vi "BeamPointing General v08.vi"() -> ()   [LabVIEW 2013]
doc: "This example illustrates how to perform a continuous acquisition with a USB camera."
uses:
  <vilib>/vision/Image Controls.llb/IMAQ Image.ctl
  <vilib>/userdefined/High Color/IMAQdx.ctl
  shared programs/GUI_Template/GUI_master/tcp_new_data_event.ctl
  shared programs/GUI_Template/GUI_master/tcp new data cluster.ctl
  Add ROI Offset ImgData.vi
  Add Or Replace Coord Array.vi
  Add Or Replace Img Array.vi
  Add ROI Offset RectFilter.vi
  Add Or Replace String Array.vi
  <vilib>/regexp/Match Regular Expression.xnode
  <vilib>/vision/NI_Vision_Development_Module.lvlib
  <resource>/objmgr/IMAQImage.rc
  <vilib>/Analysis/NI_AALBase.lvlib
  <vilib>/Analysis/NI_AALPro.lvlib
panel:
  out "image::1":T1(plugin-control) caption="Mode1"
  out "image::4":T1(plugin-control) caption="Mode1"
  out "image::5":T1(plugin-control) caption="Mode1"
  out "image::6":T1(plugin-control) caption="Mode1"
  out "image::7":T1(plugin-control) caption="Mode1"
  out "image::8":T1(plugin-control) caption="Mode1"
  out "GUIdevice 5":string="M1Cam"
  out "GUIdevice 4":string="M1Cam"
  out "GUIdevice 7":string="M1Cam"
  out "GUIdevice 6":string="M1Cam"
  out "GUIdevice 8":string="M1Cam"
  out "GUIdevice 9":string="M1Cam"
  out "image::9":T1(plugin-control) caption="Mode1"
  out "GUIdevice 3":string="M1Cam"
  out "GUIdevice 1":string="M1Cam"
  out "GUIdevice 2":string="M1Cam"
  out "image::2":T1(plugin-control) caption="Mode1"
  out "image::3":T1(plugin-control) caption="Mode1"
  out "error IO 2":errorcluster
  in  "insert tag":bool=TRUE
  out "tcp data event":T2
  in  "image prefix 2":string="gbpimage"
  in  "newMC":bool=TRUE
  out "configarraychanged":bool
  in  "Stop 2":bool
  out "image names":string[](array[string])
  out "TCP IDs":refnum<k5>[](array[refnum])
  out "Image Dst Out":T1
  in  "recenter":bool
  out "Beam Detected":bool
  out "Move Y":bool
  out "Move X":bool
  in  "LoopMode":bool caption="Mode"
  in  "rescale":bool=TRUE
  in  "Step Size":u16=5
  in  "Feedback":bool
  out "MoveInProgress":bool caption="Move In Progress"
  in  "USB cameras":i32(listbox)=1 caption="Select Camera"
  in  "Manual Move":T3={"Down"=FALSE, "Up"=FALSE, "Right"=FALSE, "Left"=FALSE, "APulses X"=200, "APulses Y"=200, "StopButton"=FALSE}
  out "Status":string
  in  "Internal controls and indicators":T4(tab)
  out "grab loop i":i32=4
  out "Image client connect errors":errorcluster[](array[cluster])
  out "Image client grab errors":errorcluster[](array[cluster])=[{"status"=TRUE, "code"=56, "source"="UDP Read in GrabImageUDP.vi->BeamPointing General v03.vi"}, {"status"=TRUE, "code"=56, "source"="UDP Read in GrabImageUDP.vi->BeamPointing General v03.vi"}, {"status"=TRUE, "code"=56, "source"="UDP Read in GrabImageUDP.vi->BeamPointing General v03.vi"}, {"status"=TRUE, "code"=56, "source"="UDP Read in GrabImageUDP.vi->BeamPointing General v03.vi"}, {"status"=TRUE, "code"=56, "source"="UDP Read in GrabImageUDP.vi->BeamPointing General v03.vi"}, {"status"=TRUE, "code"=56, "source"="UDP Read in GrabImageUDP.vi->BeamPointing General v03.vi"}]
  out "Current ImageServer":cluster{"IPAddress":string, "Port":i32}={"IPAddress"="234.5.6.8", "Port"=58445}
  out "Ann. Images":T1[](array[typedef])=["imageserver0", "imageserver1", "imageserver2", "imageserver3", "imageserver4", "imageserver5"]
  in  "Tab Control 2":enum32{"Image saving", "stats", "TCP", "cams"}(tab)=enum."cams"
  in  "Boolean":bool
  in  "Base Directory":path
  out "SaveImgError":errorcluster
  in  "SavePict":bool
  out "error CamS":errorcluster
  out "Switch Time":u32=200
  out "one loop":u32=130
  out "# imgs in buffer":i32=5
  out "ImgBufferSize":i32=5
  out "AcqTime":u32=610845
  out "State":i32=12
  out "Main processing loop i":i32=3683
  out "TCPconnecAnswer":bool=TRUE
  out "TCPconnecCmd":bool=TRUE
  out "error close connect":errorcluster
  in  "Remove Camera":bool
  in  "Mirror List Path":path=path "Z:/Software/control-common/Configuration files/DeviceList100TW.xml"
  out "XML Config File Path":path=path "Z:/Software/control-common/Configuration files/ConfigFile_192_168_10_184.xml"
  in  "USB/RS170 cams":bool=TRUE
  in  "Add Camera":bool
  out "# of cams":i32=6
  in  "# Channels on Ontrak":i32
  in  "Corr":bool[](array[boolean])=[FALSE, FALSE, FALSE, FALSE, FALSE, FALSE]
  out "Det":bool[](array[boolean])
  out "error out":errorcluster
  out "IMAQ status":bool
  out "Avg Img Buffer":u8[][][](array[numeric])
  out "Switch in":u32=299180745
  out "MirrorList":string[][](array[string])
  out "Corrective Move XY":T5(array[cluster])
  out "Cameras Names":string[](array[string])=["Null", "Null", "Null", "Null", "Null", "Null"]
  out "Deviation":cluster{"Dev. X":sgl, "Dev. Y":sgl}={"Dev. X"=0.0, "Dev. Y"=-5.0} {"Dev. X" format="%.1f"; "Dev. Y" format="%.1f"}
  out "Buffer2":T1
  out "DownloadedImg":T1
  out "CurrentName":string="*100TW M10"
  out "XML errors":bool
  out "Image Odd Out":T1
  out "DeviceNames":string[](array[string])=["no-device", "GasJet", "Godzilla_M1", "Godzilla_M2", "Godzilla_M3", "Godzilla_M4", "Godzilla_M6", "Godzilla_M8_Steer", "Chihuahua_M1", "Chihuahua_M2", "Collider_M4", "Collider_M5", "Collider_M8 Translation s3c4", "HeaterBlue-M1", "HeaterBlue-M2", "HeaterBlue-M3", "THz OAP Down", "G Spot Camera", "G Spot Monitor", "C Spot Monitor", "p15c4-Free", "THz_M5", "THz_M7A & Xtal", "THz_M7B", "THz MIrror Top", "THz OAP Top", "p2s2c2-Free", "p2s2c3-Free", "p2s2c4-Free", "Heater_M0", "Heater_M4", "Heater_M5", "Ignitor Iris", "Ignitor_M4", "Collider_M6", "Collder_M7", "C Spot Camera", "p2s5c1-FREE", "p2s5c2-FREE", "p2s5c3-FREE", "p2c5c4-FREE", "*100TW M9", "*100TW M10", "*100TW Preamp Up", "*100TW Input Preamp2", "*100TW Output Preamp2", "*100TW M0", "*100TW M2", "*100TW M4", "*100TW M6", "*100TW M8", "*100TW M13", "*100TW M20", "*100TW M22", "*100TW M23", "no pico", "no pico", "no pico", "mobile no ir", "regen out-salad#1", "preamp in-salad#2", "XPW 1", "blue periscope regen", "godzilla 1st", "godzilla IN", "Chihuahua IN", "Chihuahua 1st", "??XPW pico2", "Preamp 3rd pass", "Blue regen out"]
  out "size(s)":i32[](array[numeric])=[964, 1288]
  out "Iteration":u32
  in  "Onward":bool=TRUE
  out "Ellipse edges":cluster{"X":sgl, "Y":sgl}[](array[cluster])
  out "Buffer":T1
  out "Output Img":T1
  out "Reference Img":T1
  out "Background Img":T1
  out "counter":i32
  out "First step":bool
  out "IMAQ Session":refnum<k11>
  out "IMAQ Session Array":refnum<k11>[](array[refnum])
  out "Display Current":bool=TRUE
  out "Region of Interest":i32[](array[numeric])
  out "Acq Img":T1
  out "MoveInProgressTimeIN":u32=296721656
  out "IMAQdx Session":T6="cam2"
  out "start":u32=299180614
  out "Avg Deviation":cluster{sgl, sgl}={0.0, -5.0}
  out "InProgress":string[](array[string])
  out "Centroid Avg Buffer":cluster{"X Centroid":sgl, "Y Centroid":sgl}[](array[cluster])=[{"X Centroid"=343.0, "Y Centroid"=203.0}, {"X Centroid"=301.0, "Y Centroid"=181.0}, {"X Centroid"=334.0, "Y Centroid"=201.0}, {"X Centroid"=289.0, "Y Centroid"=154.0}, {"X Centroid"=319.0, "Y Centroid"=232.0}]
  out "Img Buffer":T1[](array[typedef])=["Buffer0", "Buffer1", "Buffer2", "Buffer3", "Buffer4"]
  out "OpenTime":u32=298569900
  out "CloseCam":bool=TRUE
  out "RunON/OFF":bool
  out "last move time":u32=281970384
  out "DeviationArray":cluster{"X Centroid":sgl, "Y Centroid":sgl}[](array[cluster])
  out "ConnectArray":T7(array[cluster])=[{"IPaddress"="192.168.10.34", "Port"=63420, "connection ID"=refnum, "TCP error"={"status"=FALSE, "code"=0, "source"=""}}, {"IPaddress"="192.168.10.184", "Port"=63430, "connection ID"=refnum, "TCP error"={"status"=FALSE, "code"=0, "source"=""}}]
  out "Raw images":T1[](array[typedef])=["imageserver0", "imageserver1", "imageserver2", "imageserver3", "imageserver4", "imageserver5"]
  in  "XML Config File Path 2":path=path "H:/Software/control-common/Configuration files/ConfigFile_192_168_10_184.xml"
  out "AddCameraCluster":T8={"Add?"=FALSE, "Channel"=6, "Device Name"="no-device"}
  out "RemoveCameraCluster":cluster{"Remove?":bool, "number":i32}={"Remove?"=FALSE, "number"=-1}
  out "NewAvg":bool
  out "Thresh Img":T1
  out "Avg Img":T1
  out "UDP connect array":refnum<k16>[](array[refnum])
  out "really save cfg?":bool
  out "Buffer3":T1
  out "CamConfigArray":T9(array[cluster])=[{"ID"=64.0, "Name"="*100TW M8", "DeviceID"={"Slot Connector"=24, "IP Adress"="192.168.10.34", "Port"=63420, "Type"="picodriver"}, "CorrectConfig Cluster"={"Detection Parameters"={"Contrast"=0, "Treshold"=0, "Max Intensity"=0, "Max Intensity%"=0, "Rx"=0, "Ry"=0, "R%"=0.0}, "Reverse"={"Reverse X"=FALSE, "Reverse Y"=FALSE}, "Target"={"X Target"=0.0, "Y Target"=0.0}, "Region of Interest"=[0, 0, 0, 0], "Correction Parameters"={"X"=0.0, "Y"=0.0, "Movement Type"=0}, "Acquisition Parameters"={"Brightness"=0.0, "Contrast"=0.0, "Saturation"=0.0, "White level"=0.0}, "Background Path"=path "", "Reference Path"=path "", "XCalibration"=[], "YCalibration"=[]}, "Ontrak Channel"=0, "IMAQdx Session 2"="cam2", "ImageServer"={"IPAddress"="234.5.6.8", "Port"=58450}}, {"ID"=55.0, "Name"="*100TW M9", "DeviceID"={"Slot Connector"=31, "IP Adress"="192.168.10.34", "Port"=63420, "Type"="picodriver"}, "CorrectConfig Cluster"={"Detection Parameters"={"Contrast"=0, "Treshold"=0, "Max Intensity"=0, "Max Intensity%"=0, "Rx"=0, "Ry"=0, "R%"=0.0}, "Reverse"={"Reverse X"=FALSE, "Reverse Y"=FALSE}, "Target"={"X Target"=631.0, "Y Target"=473.0}, "Region of Interest"=[0, 0, 0, 0], "Correction Parameters"={"X"=0.0, "Y"=0.0, "Movement Type"=0}, "Acquisition Parameters"={"Brightness"=0.0, "Contrast"=0.0, "Saturation"=0.0, "White level"=0.0}, "Background Path"=path "", "Reference Path"=path "", "XCalibration"=[], "YCalibration"=[]}, "Ontrak Channel"=0, "IMAQdx Session 2"="cam2", "ImageServer"={"IPAddress"="234.5.6.8", "Port"=58444}}, {"ID"=56.0, "Name"="*100TW M10", "DeviceID"={"Slot Connector"=32, "IP Adress"="192.168.10.34", "Port"=63420, "Type"="picodriver"}, "CorrectConfig Cluster"={"Detection Parameters"={"Contrast"=53, "Treshold"=53, "Max Intensity"=255, "Max Intensity%"=80, "Rx"=116, "Ry"=92, "R%"=50.0}, "Reverse"={"Reverse X"=FALSE, "Reverse Y"=TRUE}, "Target"={"X Target"=334.0, "Y Target"=206.0}, "Region of Interest"=[0, 0, 0, 0], "Correction Parameters"={"X"=100.0, "Y"=100.0, "Movement Type"=0}, "Acquisition Parameters"={"Brightness"=0.0, "Contrast"=0.0, "Saturation"=0.0, "White level"=0.0}, "Background Path"=path "", "Reference Path"=path "", "XCalibration"=[], "YCalibration"=[]}, "Ontrak Channel"=0, "IMAQdx Session 2"="cam2", "ImageServer"={"IPAddress"="234.5.6.8", "Port"=58445}}, {"ID"=0.0, "Name"="*100TW M20", "DeviceID"={"Slot Connector"=1, "IP Adress"="192.168.10.184", "Port"=63430, "Type"="picodriver"}, "CorrectConfig Cluster"={"Detection Parameters"={"Contrast"=66, "Treshold"=66, "Max Intensity"=255, "Max Intensity%"=80, "Rx"=30, "Ry"=30, "R%"=50.0}, "Reverse"={"Reverse X"=TRUE, "Reverse Y"=TRUE}, "Target"={"X Target"=284.6373, "Y Target"=160.1435}, "Region of Interest"=[0, 0, 0, 0], "Correction Parameters"={"X"=20.0, "Y"=20.0, "Movement Type"=0}, "Acquisition Parameters"={"Brightness"=0.0, "Contrast"=0.0, "Saturation"=0.0, "White level"=0.0}, "Background Path"=path "", "Reference Path"=path "", "XCalibration"=[{-23000.0, -242.0}, {-22000.0, -229.0}, {-21000.0, -215.0}, {-20000.0, -203.0}, {-19000.0, -192.0}, {-18000.0, -182.0}, {-17000.0, -172.0}, {-16000.0, -162.0}, {-15000.0, -153.0}, {-14000.0, -141.0}, {-13000.0, -126.0}, {-12000.0, -105.0}, {-11000.0, -77.0}, {-10000.0, -44.0}, {0.0, 4.0}, {11000.0, 98.0}, {12000.0, 109.0}, {13000.0, 119.0}, {14000.0, 130.0}, {15000.0, 140.0}, {16000.0, 151.0}, {17000.0, 161.0}, {18000.0, 171.0}, {19000.0, 182.0}, {20000.0, 193.0}, {21000.0, 205.0}, {22000.0, 217.0}, {23000.0, 229.0}], "YCalibration"=[{-23000.0, 196.0}, {-22000.0, 189.0}, {-21000.0, 182.0}, {-20000.0, 174.0}, {-19000.0, 164.0}, {-18000.0, 153.0}, {-17000.0, 141.0}, {-16000.0, 133.0}, {-15000.0, 126.0}, {-14000.0, 117.0}, {-13000.0, 105.0}, {-12000.0, 90.0}, {-11000.0, 69.0}, {-10000.0, 42.0}, {0.0, -4.0}, {11000.0, -96.0}, {12000.0, -99.0}, {13000.0, -101.0}, {14000.0, -103.0}, {15000.0, -109.0}, {16000.0, -118.0}, {17000.0, -129.0}, {18000.0, -143.0}, {19000.0, -155.0}, {20000.0, -166.0}, {21000.0, -174.0}, {22000.0, -181.0}, {23000.0, -187.0}]}, "Ontrak Channel"=0, "IMAQdx Session 2"="cam2", "ImageServer"={"IPAddress"="234.5.6.8", "Port"=58443}}, {"ID"=12.0, "Name"="*100TW M22", "DeviceID"={"Slot Connector"=3, "IP Adress"="192.168.10.184", "Port"=63430, "Type"="picodriver"}, "CorrectConfig Cluster"={"Detection Parameters"={"Contrast"=59, "Treshold"=59, "Max Intensity"=255, "Max Intensity%"=80, "Rx"=47, "Ry"=33, "R%"=50.0}, "Reverse"={"Reverse X"=FALSE, "Reverse Y"=TRUE}, "Target"={"X Target"=319.0, "Y Target"=219.0}, "Region of Interest"=[0, 0, 0, 0], "Correction Parameters"={"X"=10000.0, "Y"=10000.0, "Movement Type"=0}, "Acquisition Parameters"={"Brightness"=0.0, "Contrast"=0.0, "Saturation"=0.0, "White level"=0.0}, "Background Path"=path "", "Reference Path"=path "", "XCalibration"=[], "YCalibration"=[]}, "Ontrak Channel"=0, "IMAQdx Session 2"="cam2", "ImageServer"={"IPAddress"="234.5.6.8", "Port"=58446}}, {"ID"=12.0, "Name"="*100TW M23", "DeviceID"={"Slot Connector"=4, "IP Adress"="192.168.10.184", "Port"=63430, "Type"="picodriver"}, "CorrectConfig Cluster"={"Detection Parameters"={"Contrast"=11, "Treshold"=11, "Max Intensity"=255, "Max Intensity%"=90, "Rx"=180, "Ry"=110, "R%"=50.0}, "Reverse"={"Reverse X"=FALSE, "Reverse Y"=TRUE}, "Target"={"X Target"=303.0, "Y Target"=342.0}, "Region of Interest"=[0, 0, 0, 0], "Correction Parameters"={"X"=0.0, "Y"=0.0, "Movement Type"=0}, "Acquisition Parameters"={"Brightness"=0.0, "Contrast"=0.0, "Saturation"=0.0, "White level"=0.0}, "Background Path"=path "", "Reference Path"=path "", "XCalibration"=[], "YCalibration"=[]}, "Ontrak Channel"=0, "IMAQdx Session 2"="cam2", "ImageServer"={"IPAddress"="234.5.6.8", "Port"=58442}}] {"CorrectConfig Cluster"."Acquisition Parameters"."White level" scale=0.3..1.26 scale format="%#_2f"; "CorrectConfig Cluster"."Acquisition Parameters"."Saturation" scale=0.5..1.5 scale format="%#_3f"; "CorrectConfig Cluster"."Acquisition Parameters"."Contrast" scale=0.4..1.5 scale format="%#_3f"; "CorrectConfig Cluster"."Acquisition Parameters"."Brightness" scale=-50.0..50.0 scale format="%#_2f"; "CorrectConfig Cluster"."Correction Parameters"."Movement Type" items=["Step", "Proportionnal"]; "CorrectConfig Cluster"."Target"."X Target" format="%#_5g"; "CorrectConfig Cluster"."Target"."Y Target" format="%#_5g"; "CorrectConfig Cluster"."Detection Parameters"."Max Intensity%" max=100 step=1}
  out "Ellipse":T10 {"Minor Axis"."Point 2"."Y" format="%.2f"; "Minor Axis"."Point 2"."X" format="%.2f"; "Minor Axis"."Point 1"."Y" format="%.2f"; "Minor Axis"."Point 1"."X" format="%.2f"; "Major Axis"."Point 2"."Y" format="%.2f"; "Major Axis"."Point 2"."X" format="%.2f"; "Major Axis"."Point 1"."Y" format="%.2f"; "Major Axis"."Point 1"."X" format="%.2f"; "Center"."Y" format="%.2f"; "Center"."X" format="%.2f"}
  out "Avg Variation":cluster{"mean X":dbl, "mean Y":dbl}={"mean X"=nan, "mean Y"=nan} {"mean X" format="%#_4g"; "mean Y" format="%#_4g"}
  in  "Acquisition Parameters dx":T11 {"Parameter4" min=0.0 max=0.1 scale=0.0..0.1 scale format="%#_2f"; "Parameter3" min=0.0 max=3.0 scale=0.0..3.0 scale format="%#_3f"; "Parameter2" min=1.0 max=10.0 scale=1.0..10.0 scale format="%#_3f"; "Parameter1" min=1 max=1048576 step=1 scale=1.0..1048576.0}
  in  "set scales":bool
  out "Image Ports":i32[](array[numeric])
  out "Image IPs":string[](array[string])
  out "device associated":string
  in  "Background Path":path
  in  "Reference Path":path
  out "BestRects Cluster":T12={"PreviousCenter"={"X"=0.0, "Y"=0.0}, "CurrentCenter"={"X"=334.0, "Y"=201.0}}
  out "Default devices":string[](array[string])=["*100TW M8", "*100TW M9", "*100TW M10", "*100TW M20", "*100TW M22", "*100TW M23"]
  out "Img Size":i32[](array[numeric])=[0, 0, 1288, 964]
  out "RectFilter":T13={"Left"=257, "Top"=144, "Right"=399, "Bottom"=260, "Rotation"=10.484647750854492} {"Rotation" format="%.2f"; "Left" scale=0.0..1024.0; "Right" scale=0.0..1024.0}
  out "History XY Buffer":T14(array[cluster])
  out "ImgDataArray":T15(array[cluster])
  out "DeviceList":T16(array[cluster])=[{"ID"=0.0, "Name"="no-device", "DeviceID"={"Slot Connector"=0, "IP Adress"="Ipaddress", "Port"=0, "Type"="Type"}, "Detection Parameters"={"Contrast"=0, "Treshold"=0, "Max Intensity"=0, "Max Intensity%"=0, "Rx"=0, "Ry"=0, "R%"=0.0}, "Reverse"={"Reverse X"=FALSE, "Reverse Y"=FALSE}, "Target"={"X Target"=0.0, "Y Target"=0.0}, "Region of Interest"=[0, 0, 0, 0], "Correction Parameters"={"X"=0.0, "Y"=0.0, "Movement Type"=0}, "Acquisition Parameters"={"Brightness"=0.0, "Contrast"=0.0, "Saturation"=0.0, "White level"=0.0}, "Background Path"=path "", "Reference Path"=path "", "XCalibration"=[], "YCalibration"=[], "ImageServer"={"IPAddress"="127.0.0.1", "Port"=3500}}, {"ID"=0.0, "Name"="GasJet", "DeviceID"={"Slot Connector"=44, "IP Adress"="192.168.10.183", "Port"=63400, "Type"="picodriver"}, "Detection Parameters"={"Contrast"=0, "Treshold"=0, "Max Intensity"=0, "Max Intensity%"=0, "Rx"=0, "Ry"=0, "R%"=0.0}, "Reverse"={"Reverse X"=FALSE, "Reverse Y"=FALSE}, "Target"={"X Target"=0.0, "Y Target"=0.0}, "Region of Interest"=[0, 0, 0, 0], "Correction Parameters"={"X"=0.0, "Y"=0.0, "Movement Type"=0}, "Acquisition Parameters"={"Brightness"=0.0, "Contrast"=0.0, "Saturation"=0.0, "White level"=0.0}, "Background Path"=path "", "Reference Path"=path "", "XCalibration"=[], "YCalibration"=[], "ImageServer"={"IPAddress"="127.0.0.1", "Port"=3500}}, {"ID"=14.0, "Name"="Godzilla_M1", "DeviceID"={"Slot Connector"=11, "IP Adress"="192.168.10.183", "Port"=63400, "Type"="picodriver"}, "Detection Parameters"={"Contrast"=0, "Treshold"=0, "Max Intensity"=0, "Max Intensity%"=0, "Rx"=0, "Ry"=0, "R%"=0.0}, "Reverse"={"Reverse X"=FALSE, "Reverse Y"=FALSE}, "Target"={"X Target"=0.0, "Y Target"=0.0}, "Region of Interest"=[0, 0, 0, 0], "Correction Parameters"={"X"=0.0, "Y"=0.0, "Movement Type"=0}, "Acquisition Parameters"={"Brightness"=0.0, "Contrast"=0.0, "Saturation"=0.0, "White level"=0.0}, "Background Path"=path "", "Reference Path"=path "", "XCalibration"=[], "YCalibration"=[], "ImageServer"={"IPAddress"="127.0.0.1", "Port"=3500}}, {"ID"=15.0, "Name"="Godzilla_M2", "DeviceID"={"Slot Connector"=12, "IP Adress"="192.168.10.183", "Port"=63400, "Type"="picodriver"}, "Detection Parameters"={"Contrast"=0, "Treshold"=0, "Max Intensity"=0, "Max Intensity%"=0, "Rx"=0, "Ry"=0, "R%"=0.0}, "Reverse"={"Reverse X"=FALSE, "Reverse Y"=FALSE}, "Target"={"X Target"=0.0, "Y Target"=0.0}, "Region of Interest"=[0, 0, 0, 0], "Correction Parameters"={"X"=0.0, "Y"=0.0, "Movement Type"=0}, "Acquisition Parameters"={"Brightness"=0.0, "Contrast"=0.0, "Saturation"=0.0, "White level"=0.0}, "Background Path"=path "", "Reference Path"=path "", "XCalibration"=[], "YCalibration"=[], "ImageServer"={"IPAddress"="127.0.0.1", "Port"=3500}}, {"ID"=16.0, "Name"="Godzilla_M3", "DeviceID"={"Slot Connector"=13, "IP Adress"="192.168.10.183", "Port"=63400, "Type"="picodriver"}, "Detection Parameters"={"Contrast"=0, "Treshold"=0, "Max Intensity"=0, "Max Intensity%"=0, "Rx"=0, "Ry"=0, "R%"=0.0}, "Reverse"={"Reverse X"=FALSE, "Reverse Y"=FALSE}, "Target"={"X Target"=0.0, "Y Target"=0.0}, "Region of Interest"=[0, 0, 0, 0], "Correction Parameters"={"X"=0.0, "Y"=0.0, "Movement Type"=0}, "Acquisition Parameters"={"Brightness"=0.0, "Contrast"=0.0, "Saturation"=0.0, "White level"=0.0}, "Background Path"=path "", "Reference Path"=path "", "XCalibration"=[], "YCalibration"=[], "ImageServer"={"IPAddress"="127.0.0.1", "Port"=3500}}, {"ID"=17.0, "Name"="Godzilla_M4", "DeviceID"={"Slot Connector"=14, "IP Adress"="192.168.10.183", "Port"=63400, "Type"="picodriver"}, "Detection Parameters"={"Contrast"=0, "Treshold"=0, "Max Intensity"=0, "Max Intensity%"=0, "Rx"=0, "Ry"=0, "R%"=0.0}, "Reverse"={"Reverse X"=FALSE, "Reverse Y"=FALSE}, "Target"={"X Target"=0.0, "Y Target"=0.0}, "Region of Interest"=[0, 0, 0, 0], "Correction Parameters"={"X"=0.0, "Y"=0.0, "Movement Type"=0}, "Acquisition Parameters"={"Brightness"=0.0, "Contrast"=0.0, "Saturation"=0.0, "White level"=0.0}, "Background Path"=path "", "Reference Path"=path "", "XCalibration"=[], "YCalibration"=[], "ImageServer"={"IPAddress"="127.0.0.1", "Port"=3500}}, {"ID"=18.0, "Name"="Godzilla_M6", "DeviceID"={"Slot Connector"=21, "IP Adress"="192.168.10.183", "Port"=63400, "Type"="picodriver"}, "Detection Parameters"={"Contrast"=0, "Treshold"=0, "Max Intensity"=0, "Max Intensity%"=0, "Rx"=0, "Ry"=0, "R%"=0.0}, "Reverse"={"Reverse X"=FALSE, "Reverse Y"=FALSE}, "Target"={"X Target"=0.0, "Y Target"=0.0}, "Region of Interest"=[0, 0, 0, 0], "Correction Parameters"={"X"=0.0, "Y"=0.0, "Movement Type"=0}, "Acquisition Parameters"={"Brightness"=0.0, "Contrast"=0.0, "Saturation"=0.0, "White level"=0.0}, "Background Path"=path "", "Reference Path"=path "", "XCalibration"=[], "YCalibration"=[], "ImageServer"={"IPAddress"="127.0.0.1", "Port"=3500}}, {"ID"=19.0, "Name"="Godzilla_M8_Steer", "DeviceID"={"Slot Connector"=22, "IP Adress"="192.168.10.183", "Port"=63400, "Type"="picodriver"}, "Detection Parameters"={"Contrast"=0, "Treshold"=0, "Max Intensity"=0, "Max Intensity%"=0, "Rx"=0, "Ry"=0, "R%"=0.0}, "Reverse"={"Reverse X"=FALSE, "Reverse Y"=FALSE}, "Target"={"X Target"=0.0, "Y Target"=0.0}, "Region of Interest"=[0, 0, 0, 0], "Correction Parameters"={"X"=0.0, "Y"=0.0, "Movement Type"=0}, "Acquisition Parameters"={"Brightness"=0.0, "Contrast"=0.0, "Saturation"=0.0, "White level"=0.0}, "Background Path"=path "", "Reference Path"=path "", "XCalibration"=[], "YCalibration"=[], "ImageServer"={"IPAddress"="127.0.0.1", "Port"=3500}}, {"ID"=20.0, "Name"="Chihuahua_M1", "DeviceID"={"Slot Connector"=23, "IP Adress"="192.168.10.183", "Port"=63400, "Type"="picodriver"}, "Detection Parameters"={"Contrast"=0, "Treshold"=0, "Max Intensity"=0, "Max Intensity%"=0, "Rx"=0, "Ry"=0, "R%"=0.0}, "Reverse"={"Reverse X"=FALSE, "Reverse Y"=FALSE}, "Target"={"X Target"=0.0, "Y Target"=0.0}, "Region of Interest"=[0, 0, 0, 0], "Correction Parameters"={"X"=0.0, "Y"=0.0, "Movement Type"=0}, "Acquisition Parameters"={"Brightness"=0.0, "Contrast"=0.0, "Saturation"=0.0, "White level"=0.0}, "Background Path"=path "", "Reference Path"=path "", "XCalibration"=[], "YCalibration"=[], "ImageServer"={"IPAddress"="127.0.0.1", "Port"=3500}}, {"ID"=21.0, "Name"="Chihuahua_M2", "DeviceID"={"Slot Connector"=24, "IP Adress"="192.168.10.183", "Port"=63400, "Type"="picodriver"}, "Detection Parameters"={"Contrast"=0, "Treshold"=0, "Max Intensity"=0, "Max Intensity%"=0, "Rx"=0, "Ry"=0, "R%"=0.0}, "Reverse"={"Reverse X"=FALSE, "Reverse Y"=FALSE}, "Target"={"X Target"=0.0, "Y Target"=0.0}, "Region of Interest"=[0, 0, 0, 0], "Correction Parameters"={"X"=0.0, "Y"=0.0, "Movement Type"=0}, "Acquisition Parameters"={"Brightness"=0.0, "Contrast"=0.0, "Saturation"=0.0, "White level"=0.0}, "Background Path"=path "", "Reference Path"=path "", "XCalibration"=[], "YCalibration"=[], "ImageServer"={"IPAddress"="127.0.0.1", "Port"=3500}}, {"ID"=22.0, "Name"="Collider_M4", "DeviceID"={"Slot Connector"=31, "IP Adress"="192.168.10.183", "Port"=63400, "Type"="picodriver"}, "Detection Parameters"={"Contrast"=0, "Treshold"=0, "Max Intensity"=0, "Max Intensity%"=0, "Rx"=0, "Ry"=0, "R%"=0.0}, "Reverse"={"Reverse X"=FALSE, "Reverse Y"=FALSE}, "Target"={"X Target"=0.0, "Y Target"=0.0}, "Region of Interest"=[0, 0, 0, 0], "Correction Parameters"={"X"=0.0, "Y"=0.0, "Movement Type"=0}, "Acquisition Parameters"={"Brightness"=0.0, "Contrast"=0.0, "Saturation"=0.0, "White level"=0.0}, "Background Path"=path "", "Reference Path"=path "", "XCalibration"=[], "YCalibration"=[], "ImageServer"={"IPAddress"="127.0.0.1", "Port"=3500}}, {"ID"=23.0, "Name"="Collider_M5", "DeviceID"={"Slot Connector"=32, "IP Adress"="192.168.10.183", "Port"=63400, "Type"="picodriver"}, "Detection Parameters"={"Contrast"=0, "Treshold"=0, "Max Intensity"=0, "Max Intensity%"=0, "Rx"=0, "Ry"=0, "R%"=0.0}, "Reverse"={"Reverse X"=FALSE, "Reverse Y"=FALSE}, "Target"={"X Target"=0.0, "Y Target"=0.0}, "Region of Interest"=[0, 0, 0, 0], "Correction Parameters"={"X"=0.0, "Y"=0.0, "Movement Type"=0}, "Acquisition Parameters"={"Brightness"=0.0, "Contrast"=0.0, "Saturation"=0.0, "White level"=0.0}, "Background Path"=path "", "Reference Path"=path "", "XCalibration"=[], "YCalibration"=[], "ImageServer"={"IPAddress"="127.0.0.1", "Port"=3500}}, {"ID"=24.0, "Name"="Collider_M8 Translation s3c4", "DeviceID"={"Slot Connector"=33, "IP Adress"="192.168.10.183", "Port"=63400, "Type"="picodriver"}, "Detection Parameters"={"Contrast"=0, "Treshold"=0, "Max Intensity"=0, "Max Intensity%"=0, "Rx"=0, "Ry"=0, "R%"=0.0}, "Reverse"={"Reverse X"=FALSE, "Reverse Y"=FALSE}, "Target"={"X Target"=0.0, "Y Target"=0.0}, "Region of Interest"=[0, 0, 0, 0], "Correction Parameters"={"X"=0.0, "Y"=0.0, "Movement Type"=0}, "Acquisition Parameters"={"Brightness"=0.0, "Contrast"=0.0, "Saturation"=0.0, "White level"=0.0}, "Background Path"=path "", "Reference Path"=path "", "XCalibration"=[], "YCalibration"=[], "ImageServer"={"IPAddress"="127.0.0.1", "Port"=3500}}, {"ID"=26.0, "Name"="HeaterBlue-M1", "DeviceID"={"Slot Connector"=34, "IP Adress"="192.168.10.183", "Port"=63400, "Type"="picodriver"}, "Detection Parameters"={"Contrast"=0, "Treshold"=0, "Max Intensity"=0, "Max Intensity%"=0, "Rx"=0, "Ry"=0, "R%"=0.0}, "Reverse"={"Reverse X"=FALSE, "Reverse Y"=FALSE}, "Target"={"X Target"=0.0, "Y Target"=0.0}, "Region of Interest"=[0, 0, 0, 0], "Correction Parameters"={"X"=0.0, "Y"=0.0, "Movement Type"=0}, "Acquisition Parameters"={"Brightness"=0.0, "Contrast"=0.0, "Saturation"=0.0, "White level"=0.0}, "Background Path"=path "", "Reference Path"=path "", "XCalibration"=[], "YCalibration"=[], "ImageServer"={"IPAddress"="127.0.0.1", "Port"=3500}}, {"ID"=27.0, "Name"="HeaterBlue-M2", "DeviceID"={"Slot Connector"=41, "IP Adress"="192.168.10.183", "Port"=63400, "Type"="picodriver"}, "Detection Parameters"={"Contrast"=0, "Treshold"=0, "Max Intensity"=0, "Max Intensity%"=0, "Rx"=0, "Ry"=0, "R%"=0.0}, "Reverse"={"Reverse X"=FALSE, "Reverse Y"=FALSE}, "Target"={"X Target"=0.0, "Y Target"=0.0}, "Region of Interest"=[0, 0, 0, 0], "Correction Parameters"={"X"=0.0, "Y"=0.0, "Movement Type"=0}, "Acquisition Parameters"={"Brightness"=0.0, "Contrast"=0.0, "Saturation"=0.0, "White level"=0.0}, "Background Path"=path "", "Reference Path"=path "", "XCalibration"=[], "YCalibration"=[], "ImageServer"={"IPAddress"="127.0.0.1", "Port"=3500}}, {"ID"=28.0, "Name"="HeaterBlue-M3", "DeviceID"={"Slot Connector"=42, "IP Adress"="192.168.10.183", "Port"=63400, "Type"="picodriver"}, "Detection Parameters"={"Contrast"=0, "Treshold"=0, "Max Intensity"=0, "Max Intensity%"=0, "Rx"=0, "Ry"=0, "R%"=0.0}, "Reverse"={"Reverse X"=FALSE, "Reverse Y"=FALSE}, "Target"={"X Target"=0.0, "Y Target"=0.0}, "Region of Interest"=[0, 0, 0, 0], "Correction Parameters"={"X"=0.0, "Y"=0.0, "Movement Type"=0}, "Acquisition Parameters"={"Brightness"=0.0, "Contrast"=0.0, "Saturation"=0.0, "White level"=0.0}, "Background Path"=path "", "Reference Path"=path "", "XCalibration"=[], "YCalibration"=[], "ImageServer"={"IPAddress"="127.0.0.1", "Port"=3500}}, {"ID"=29.0, "Name"="THz OAP Down", "DeviceID"={"Slot Connector"=43, "IP Adress"="192.168.10.183", "Port"=63400, "Type"="picodriver"}, "Detection Parameters"={"Contrast"=0, "Treshold"=0, "Max Intensity"=0, "Max Intensity%"=0, "Rx"=0, "Ry"=0, "R%"=0.0}, "Reverse"={"Reverse X"=FALSE, "Reverse Y"=FALSE}, "Target"={"X Target"=0.0, "Y Target"=0.0}, "Region of Interest"=[0, 0, 0, 0], "Correction Parameters"={"X"=0.0, "Y"=0.0, "Movement Type"=0}, "Acquisition Parameters"={"Brightness"=0.0, "Contrast"=0.0, "Saturation"=0.0, "White level"=0.0}, "Background Path"=path "", "Reference Path"=path "", "XCalibration"=[], "YCalibration"=[], "ImageServer"={"IPAddress"="127.0.0.1", "Port"=3500}}, {"ID"=30.0, "Name"="G Spot Camera", "DeviceID"={"Slot Connector"=51, "IP Adress"="192.168.10.183", "Port"=63400, "Type"="picodriver"}, "Detection Parameters"={"Contrast"=0, "Treshold"=0, "Max Intensity"=0, "Max Intensity%"=0, "Rx"=0, "Ry"=0, "R%"=0.0}, "Reverse"={"Reverse X"=FALSE, "Reverse Y"=FALSE}, "Target"={"X Target"=0.0, "Y Target"=0.0}, "Region of Interest"=[0, 0, 0, 0], "Correction Parameters"={"X"=0.0, "Y"=0.0, "Movement Type"=0}, "Acquisition Parameters"={"Brightness"=0.0, "Contrast"=0.0, "Saturation"=0.0, "White level"=0.0}, "Background Path"=path "", "Reference Path"=path "", "XCalibration"=[], "YCalibration"=[], "ImageServer"={"IPAddress"="127.0.0.1", "Port"=3500}}, {"ID"=31.0, "Name"="G Spot Monitor", "DeviceID"={"Slot Connector"=52, "IP Adress"="192.168.10.183", "Port"=63400, "Type"="picodriver"}, "Detection Parameters"={"Contrast"=0, "Treshold"=0, "Max Intensity"=0, "Max Intensity%"=0, "Rx"=0, "Ry"=0, "R%"=0.0}, "Reverse"={"Reverse X"=FALSE, "Reverse Y"=FALSE}, "Target"={"X Target"=0.0, "Y Target"=0.0}, "Region of Interest"=[0, 0, 0, 0], "Correction Parameters"={"X"=0.0, "Y"=0.0, "Movement Type"=0}, "Acquisition Parameters"={"Brightness"=0.0, "Contrast"=0.0, "Saturation"=0.0, "White level"=0.0}, "Background Path"=path "", "Reference Path"=path "", "XCalibration"=[], "YCalibration"=[], "ImageServer"={"IPAddress"="127.0.0.1", "Port"=3500}}, {"ID"=32.0, "Name"="C Spot Monitor", "DeviceID"={"Slot Connector"=53, "IP Adress"="192.168.10.183", "Port"=63400, "Type"="picodriver"}, "Detection Parameters"={"Contrast"=0, "Treshold"=0, "Max Intensity"=0, "Max Intensity%"=0, "Rx"=0, "Ry"=0, "R%"=0.0}, "Reverse"={"Reverse X"=FALSE, "Reverse Y"=FALSE}, "Target"={"X Target"=0.0, "Y Target"=0.0}, "Region of Interest"=[0, 0, 0, 0], "Correction Parameters"={"X"=0.0, "Y"=0.0, "Movement Type"=0}, "Acquisition Parameters"={"Brightness"=0.0, "Contrast"=0.0, "Saturation"=0.0, "White level"=0.0}, "Background Path"=path "", "Reference Path"=path "", "XCalibration"=[], "YCalibration"=[], "ImageServer"={"IPAddress"="127.0.0.1", "Port"=3500}}, {"ID"=33.0, "Name"="p15c4-Free", "DeviceID"={"Slot Connector"=54, "IP Adress"="192.168.10.183", "Port"=63400, "Type"="picodriver"}, "Detection Parameters"={"Contrast"=0, "Treshold"=0, "Max Intensity"=0, "Max Intensity%"=0, "Rx"=0, "Ry"=0, "R%"=0.0}, "Reverse"={"Reverse X"=FALSE, "Reverse Y"=FALSE}, "Target"={"X Target"=0.0, "Y Target"=0.0}, "Region of Interest"=[0, 0, 0, 0], "Correction Parameters"={"X"=0.0, "Y"=0.0, "Movement Type"=0}, "Acquisition Parameters"={"Brightness"=0.0, "Contrast"=0.0, "Saturation"=0.0, "White level"=0.0}, "Background Path"=path "", "Reference Path"=path "", "XCalibration"=[], "YCalibration"=[], "ImageServer"={"IPAddress"="127.0.0.1", "Port"=3500}}, {"ID"=34.0, "Name"="THz_M5", "DeviceID"={"Slot Connector"=11, "IP Adress"="192.168.10.183", "Port"=63410, "Type"="picodriver"}, "Detection Parameters"={"Contrast"=0, "Treshold"=0, "Max Intensity"=0, "Max Intensity%"=0, "Rx"=0, "Ry"=0, "R%"=0.0}, "Reverse"={"Reverse X"=FALSE, "Reverse Y"=FALSE}, "Target"={"X Target"=0.0, "Y Target"=0.0}, "Region of Interest"=[0, 0, 0, 0], "Correction Parameters"={"X"=0.0, "Y"=0.0, "Movement Type"=0}, "Acquisition Parameters"={"Brightness"=0.0, "Contrast"=0.0, "Saturation"=0.0, "White level"=0.0}, "Background Path"=path "", "Reference Path"=path "", "XCalibration"=[], "YCalibration"=[], "ImageServer"={"IPAddress"="127.0.0.1", "Port"=3500}}, {"ID"=35.0, "Name"="THz_M7A & Xtal", "DeviceID"={"Slot Connector"=12, "IP Adress"="192.168.10.183", "Port"=63410, "Type"="picodriver"}, "Detection Parameters"={"Contrast"=0, "Treshold"=0, "Max Intensity"=0, "Max Intensity%"=0, "Rx"=0, "Ry"=0, "R%"=0.0}, "Reverse"={"Reverse X"=FALSE, "Reverse Y"=FALSE}, "Target"={"X Target"=0.0, "Y Target"=0.0}, "Region of Interest"=[0, 0, 0, 0], "Correction Parameters"={"X"=0.0, "Y"=0.0, "Movement Type"=0}, "Acquisition Parameters"={"Brightness"=0.0, "Contrast"=0.0, "Saturation"=0.0, "White level"=0.0}, "Background Path"=path "", "Reference Path"=path "", "XCalibration"=[], "YCalibration"=[], "ImageServer"={"IPAddress"="127.0.0.1", "Port"=3500}}, {"ID"=36.0, "Name"="THz_M7B", "DeviceID"={"Slot Connector"=13, "IP Adress"="192.168.10.183", "Port"=63410, "Type"="picodriver"}, "Detection Parameters"={"Contrast"=0, "Treshold"=0, "Max Intensity"=0, "Max Intensity%"=0, "Rx"=0, "Ry"=0, "R%"=0.0}, "Reverse"={"Reverse X"=FALSE, "Reverse Y"=FALSE}, "Target"={"X Target"=0.0, "Y Target"=0.0}, "Region of Interest"=[0, 0, 0, 0], "Correction Parameters"={"X"=0.0, "Y"=0.0, "Movement Type"=0}, "Acquisition Parameters"={"Brightness"=0.0, "Contrast"=0.0, "Saturation"=0.0, "White level"=0.0}, "Background Path"=path "", "Reference Path"=path "", "XCalibration"=[], "YCalibration"=[], "ImageServer"={"IPAddress"="127.0.0.1", "Port"=3500}}, {"ID"=37.0, "Name"="THz MIrror Top", "DeviceID"={"Slot Connector"=14, "IP Adress"="192.168.10.183", "Port"=63410, "Type"="picodriver"}, "Detection Parameters"={"Contrast"=0, "Treshold"=0, "Max Intensity"=0, "Max Intensity%"=0, "Rx"=0, "Ry"=0, "R%"=0.0}, "Reverse"={"Reverse X"=FALSE, "Reverse Y"=FALSE}, "Target"={"X Target"=0.0, "Y Target"=0.0}, "Region of Interest"=[0, 0, 0, 0], "Correction Parameters"={"X"=0.0, "Y"=0.0, "Movement Type"=0}, "Acquisition Parameters"={"Brightness"=0.0, "Contrast"=0.0, "Saturation"=0.0, "White level"=0.0}, "Background Path"=path "", "Reference Path"=path "", "XCalibration"=[], "YCalibration"=[], "ImageServer"={"IPAddress"="127.0.0.1", "Port"=3500}}, {"ID"=38.0, "Name"="THz OAP Top", "DeviceID"={"Slot Connector"=21, "IP Adress"="192.168.10.183", "Port"=63410, "Type"="picodriver"}, "Detection Parameters"={"Contrast"=0, "Treshold"=0, "Max Intensity"=0, "Max Intensity%"=0, "Rx"=0, "Ry"=0, "R%"=0.0}, "Reverse"={"Reverse X"=FALSE, "Reverse Y"=FALSE}, "Target"={"X Target"=0.0, "Y Target"=0.0}, "Region of Interest"=[0, 0, 0, 0], "Correction Parameters"={"X"=0.0, "Y"=0.0, "Movement Type"=0}, "Acquisition Parameters"={"Brightness"=0.0, "Contrast"=0.0, "Saturation"=0.0, "White level"=0.0}, "Background Path"=path "", "Reference Path"=path "", "XCalibration"=[], "YCalibration"=[], "ImageServer"={"IPAddress"="127.0.0.1", "Port"=3500}}, {"ID"=39.0, "Name"="p2s2c2-Free", "DeviceID"={"Slot Connector"=22, "IP Adress"="192.168.10.183", "Port"=63410, "Type"="picodriver"}, "Detection Parameters"={"Contrast"=0, "Treshold"=0, "Max Intensity"=0, "Max Intensity%"=0, "Rx"=0, "Ry"=0, "R%"=0.0}, "Reverse"={"Reverse X"=FALSE, "Reverse Y"=FALSE}, "Target"={"X Target"=0.0, "Y Target"=0.0}, "Region of Interest"=[0, 0, 0, 0], "Correction Parameters"={"X"=0.0, "Y"=0.0, "Movement Type"=0}, "Acquisition Parameters"={"Brightness"=0.0, "Contrast"=0.0, "Saturation"=0.0, "White level"=0.0}, "Background Path"=path "", "Reference Path"=path "", "XCalibration"=[], "YCalibration"=[], "ImageServer"={"IPAddress"="127.0.0.1", "Port"=3500}}, {"ID"=40.0, "Name"="p2s2c3-Free", "DeviceID"={"Slot Connector"=23, "IP Adress"="192.168.10.183", "Port"=63410, "Type"="picodriver"}, "Detection Parameters"={"Contrast"=0, "Treshold"=0, "Max Intensity"=0, "Max Intensity%"=0, "Rx"=0, "Ry"=0, "R%"=0.0}, "Reverse"={"Reverse X"=FALSE, "Reverse Y"=FALSE}, "Target"={"X Target"=0.0, "Y Target"=0.0}, "Region of Interest"=[0, 0, 0, 0], "Correction Parameters"={"X"=0.0, "Y"=0.0, "Movement Type"=0}, "Acquisition Parameters"={"Brightness"=0.0, "Contrast"=0.0, "Saturation"=0.0, "White level"=0.0}, "Background Path"=path "", "Reference Path"=path "", "XCalibration"=[], "YCalibration"=[], "ImageServer"={"IPAddress"="127.0.0.1", "Port"=3500}}, {"ID"=41.0, "Name"="p2s2c4-Free", "DeviceID"={"Slot Connector"=24, "IP Adress"="192.168.10.183", "Port"=63410, "Type"="picodriver"}, "Detection Parameters"={"Contrast"=0, "Treshold"=0, "Max Intensity"=0, "Max Intensity%"=0, "Rx"=0, "Ry"=0, "R%"=0.0}, "Reverse"={"Reverse X"=FALSE, "Reverse Y"=FALSE}, "Target"={"X Target"=0.0, "Y Target"=0.0}, "Region of Interest"=[0, 0, 0, 0], "Correction Parameters"={"X"=0.0, "Y"=0.0, "Movement Type"=0}, "Acquisition Parameters"={"Brightness"=0.0, "Contrast"=0.0, "Saturation"=0.0, "White level"=0.0}, "Background Path"=path "", "Reference Path"=path "", "XCalibration"=[], "YCalibration"=[], "ImageServer"={"IPAddress"="127.0.0.1", "Port"=3500}}, {"ID"=42.0, "Name"="Heater_M0", "DeviceID"={"Slot Connector"=31, "IP Adress"="192.168.10.183", "Port"=63410, "Type"="picodriver"}, "Detection Parameters"={"Contrast"=0, "Treshold"=0, "Max Intensity"=0, "Max Intensity%"=0, "Rx"=0, "Ry"=0, "R%"=0.0}, "Reverse"={"Reverse X"=FALSE, "Reverse Y"=FALSE}, "Target"={"X Target"=0.0, "Y Target"=0.0}, "Region of Interest"=[0, 0, 0, 0], "Correction Parameters"={"X"=0.0, "Y"=0.0, "Movement Type"=0}, "Acquisition Parameters"={"Brightness"=0.0, "Contrast"=0.0, "Saturation"=0.0, "White level"=0.0}, "Background Path"=path "", "Reference Path"=path "", "XCalibration"=[], "YCalibration"=[], "ImageServer"={"IPAddress"="127.0.0.1", "Port"=3500}}, {"ID"=43.0, "Name"="Heater_M4", "DeviceID"={"Slot Connector"=32, "IP Adress"="192.168.10.183", "Port"=63410, "Type"="picodriver"}, "Detection Parameters"={"Contrast"=0, "Treshold"=0, "Max Intensity"=0, "Max Intensity%"=0, "Rx"=0, "Ry"=0, "R%"=0.0}, "Reverse"={"Reverse X"=FALSE, "Reverse Y"=FALSE}, "Target"={"X Target"=0.0, "Y Target"=0.0}, "Region of Interest"=[0, 0, 0, 0], "Correction Parameters"={"X"=0.0, "Y"=0.0, "Movement Type"=0}, "Acquisition Parameters"={"Brightness"=0.0, "Contrast"=0.0, "Saturation"=0.0, "White level"=0.0}, "Background Path"=path "", "Reference Path"=path "", "XCalibration"=[], "YCalibration"=[], "ImageServer"={"IPAddress"="127.0.0.1", "Port"=3500}}, {"ID"=44.0, "Name"="Heater_M5", "DeviceID"={"Slot Connector"=33, "IP Adress"="192.168.10.183", "Port"=63410, "Type"="picodriver"}, "Detection Parameters"={"Contrast"=0, "Treshold"=0, "Max Intensity"=0, "Max Intensity%"=0, "Rx"=0, "Ry"=0, "R%"=0.0}, "Reverse"={"Reverse X"=FALSE, "Reverse Y"=FALSE}, "Target"={"X Target"=0.0, "Y Target"=0.0}, "Region of Interest"=[0, 0, 0, 0], "Correction Parameters"={"X"=0.0, "Y"=0.0, "Movement Type"=0}, "Acquisition Parameters"={"Brightness"=0.0, "Contrast"=0.0, "Saturation"=0.0, "White level"=0.0}, "Background Path"=path "", "Reference Path"=path "", "XCalibration"=[], "YCalibration"=[], "ImageServer"={"IPAddress"="127.0.0.1", "Port"=3500}}, {"ID"=45.0, "Name"="Ignitor Iris", "DeviceID"={"Slot Connector"=34, "IP Adress"="192.168.10.183", "Port"=63410, "Type"="picodriver"}, "Detection Parameters"={"Contrast"=0, "Treshold"=0, "Max Intensity"=0, "Max Intensity%"=0, "Rx"=0, "Ry"=0, "R%"=0.0}, "Reverse"={"Reverse X"=FALSE, "Reverse Y"=FALSE}, "Target"={"X Target"=0.0, "Y Target"=0.0}, "Region of Interest"=[0, 0, 0, 0], "Correction Parameters"={"X"=0.0, "Y"=0.0, "Movement Type"=0}, "Acquisition Parameters"={"Brightness"=0.0, "Contrast"=0.0, "Saturation"=0.0, "White level"=0.0}, "Background Path"=path "", "Reference Path"=path "", "XCalibration"=[], "YCalibration"=[], "ImageServer"={"IPAddress"="127.0.0.1", "Port"=3500}}, {"ID"=46.0, "Name"="Ignitor_M4", "DeviceID"={"Slot Connector"=41, "IP Adress"="192.168.10.183", "Port"=63410, "Type"="picodriver"}, "Detection Parameters"={"Contrast"=0, "Treshold"=0, "Max Intensity"=0, "Max Intensity%"=0, "Rx"=0, "Ry"=0, "R%"=0.0}, "Reverse"={"Reverse X"=FALSE, "Reverse Y"=FALSE}, "Target"={"X Target"=0.0, "Y Target"=0.0}, "Region of Interest"=[0, 0, 0, 0], "Correction Parameters"={"X"=0.0, "Y"=0.0, "Movement Type"=0}, "Acquisition Parameters"={"Brightness"=0.0, "Contrast"=0.0, "Saturation"=0.0, "White level"=0.0}, "Background Path"=path "", "Reference Path"=path "", "XCalibration"=[], "YCalibration"=[], "ImageServer"={"IPAddress"="127.0.0.1", "Port"=3500}}, {"ID"=47.0, "Name"="Collider_M6", "DeviceID"={"Slot Connector"=42, "IP Adress"="192.168.10.183", "Port"=63410, "Type"="picodriver"}, "Detection Parameters"={"Contrast"=0, "Treshold"=0, "Max Intensity"=0, "Max Intensity%"=0, "Rx"=0, "Ry"=0, "R%"=0.0}, "Reverse"={"Reverse X"=FALSE, "Reverse Y"=FALSE}, "Target"={"X Target"=0.0, "Y Target"=0.0}, "Region of Interest"=[0, 0, 0, 0], "Correction Parameters"={"X"=0.0, "Y"=0.0, "Movement Type"=0}, "Acquisition Parameters"={"Brightness"=0.0, "Contrast"=0.0, "Saturation"=0.0, "White level"=0.0}, "Background Path"=path "", "Reference Path"=path "", "XCalibration"=[], "YCalibration"=[], "ImageServer"={"IPAddress"="127.0.0.1", "Port"=3500}}, {"ID"=48.0, "Name"="Collder_M7", "DeviceID"={"Slot Connector"=43, "IP Adress"="192.168.10.183", "Port"=63410, "Type"="picodriver"}, "Detection Parameters"={"Contrast"=0, "Treshold"=0, "Max Intensity"=0, "Max Intensity%"=0, "Rx"=0, "Ry"=0, "R%"=0.0}, "Reverse"={"Reverse X"=FALSE, "Reverse Y"=FALSE}, "Target"={"X Target"=0.0, "Y Target"=0.0}, "Region of Interest"=[0, 0, 0, 0], "Correction Parameters"={"X"=0.0, "Y"=0.0, "Movement Type"=0}, "Acquisition Parameters"={"Brightness"=0.0, "Contrast"=0.0, "Saturation"=0.0, "White level"=0.0}, "Background Path"=path "", "Reference Path"=path "", "XCalibration"=[], "YCalibration"=[], "ImageServer"={"IPAddress"="127.0.0.1", "Port"=3500}}, {"ID"=49.0, "Name"="C Spot Camera", "DeviceID"={"Slot Connector"=44, "IP Adress"="192.168.10.183", "Port"=63410, "Type"="picodriver"}, "Detection Parameters"={"Contrast"=0, "Treshold"=0, "Max Intensity"=0, "Max Intensity%"=0, "Rx"=0, "Ry"=0, "R%"=0.0}, "Reverse"={"Reverse X"=FALSE, "Reverse Y"=FALSE}, "Target"={"X Target"=0.0, "Y Target"=0.0}, "Region of Interest"=[0, 0, 0, 0], "Correction Parameters"={"X"=0.0, "Y"=0.0, "Movement Type"=0}, "Acquisition Parameters"={"Brightness"=0.0, "Contrast"=0.0, "Saturation"=0.0, "White level"=0.0}, "Background Path"=path "", "Reference Path"=path "", "XCalibration"=[], "YCalibration"=[], "ImageServer"={"IPAddress"="127.0.0.1", "Port"=3500}}, {"ID"=50.0, "Name"="p2s5c1-FREE", "DeviceID"={"Slot Connector"=51, "IP Adress"="192.168.10.183", "Port"=63410, "Type"="picodriver"}, "Detection Parameters"={"Contrast"=0, "Treshold"=0, "Max Intensity"=0, "Max Intensity%"=0, "Rx"=0, "Ry"=0, "R%"=0.0}, "Reverse"={"Reverse X"=FALSE, "Reverse Y"=FALSE}, "Target"={"X Target"=0.0, "Y Target"=0.0}, "Region of Interest"=[0, 0, 0, 0], "Correction Parameters"={"X"=0.0, "Y"=0.0, "Movement Type"=0}, "Acquisition Parameters"={"Brightness"=0.0, "Contrast"=0.0, "Saturation"=0.0, "White level"=0.0}, "Background Path"=path "", "Reference Path"=path "", "XCalibration"=[], "YCalibration"=[], "ImageServer"={"IPAddress"="127.0.0.1", "Port"=3500}}, {"ID"=51.0, "Name"="p2s5c2-FREE", "DeviceID"={"Slot Connector"=52, "IP Adress"="192.168.10.183", "Port"=63410, "Type"="picodriver"}, "Detection Parameters"={"Contrast"=0, "Treshold"=0, "Max Intensity"=0, "Max Intensity%"=0, "Rx"=0, "Ry"=0, "R%"=0.0}, "Reverse"={"Reverse X"=FALSE, "Reverse Y"=FALSE}, "Target"={"X Target"=0.0, "Y Target"=0.0}, "Region of Interest"=[0, 0, 0, 0], "Correction Parameters"={"X"=0.0, "Y"=0.0, "Movement Type"=0}, "Acquisition Parameters"={"Brightness"=0.0, "Contrast"=0.0, "Saturation"=0.0, "White level"=0.0}, "Background Path"=path "", "Reference Path"=path "", "XCalibration"=[], "YCalibration"=[], "ImageServer"={"IPAddress"="127.0.0.1", "Port"=3500}}, {"ID"=52.0, "Name"="p2s5c3-FREE", "DeviceID"={"Slot Connector"=53, "IP Adress"="192.168.10.183", "Port"=63410, "Type"="picodriver"}, "Detection Parameters"={"Contrast"=0, "Treshold"=0, "Max Intensity"=0, "Max Intensity%"=0, "Rx"=0, "Ry"=0, "R%"=0.0}, "Reverse"={"Reverse X"=FALSE, "Reverse Y"=FALSE}, "Target"={"X Target"=0.0, "Y Target"=0.0}, "Region of Interest"=[0, 0, 0, 0], "Correction Parameters"={"X"=0.0, "Y"=0.0, "Movement Type"=0}, "Acquisition Parameters"={"Brightness"=0.0, "Contrast"=0.0, "Saturation"=0.0, "White level"=0.0}, "Background Path"=path "", "Reference Path"=path "", "XCalibration"=[], "YCalibration"=[], "ImageServer"={"IPAddress"="127.0.0.1", "Port"=3500}}, {"ID"=53.0, "Name"="p2c5c4-FREE", "DeviceID"={"Slot Connector"=54, "IP Adress"="192.168.10.183", "Port"=63410, "Type"="picodriver"}, "Detection Parameters"={"Contrast"=0, "Treshold"=0, "Max Intensity"=0, "Max Intensity%"=0, "Rx"=0, "Ry"=0, "R%"=0.0}, "Reverse"={"Reverse X"=FALSE, "Reverse Y"=FALSE}, "Target"={"X Target"=0.0, "Y Target"=0.0}, "Region of Interest"=[0, 0, 0, 0], "Correction Parameters"={"X"=0.0, "Y"=0.0, "Movement Type"=0}, "Acquisition Parameters"={"Brightness"=0.0, "Contrast"=0.0, "Saturation"=0.0, "White level"=0.0}, "Background Path"=path "", "Reference Path"=path "", "XCalibration"=[], "YCalibration"=[], "ImageServer"={"IPAddress"="127.0.0.1", "Port"=3500}}, {"ID"=55.0, "Name"="*100TW M9", "DeviceID"={"Slot Connector"=31, "IP Adress"="192.168.10.34", "Port"=63420, "Type"="picodriver"}, "Detection Parameters"={"Contrast"=0, "Treshold"=0, "Max Intensity"=0, "Max Intensity%"=0, "Rx"=0, "Ry"=0, "R%"=0.0}, "Reverse"={"Reverse X"=FALSE, "Reverse Y"=FALSE}, "Target"={"X Target"=631.0, "Y Target"=473.0}, "Region of Interest"=[0, 0, 0, 0], "Correction Parameters"={"X"=0.0, "Y"=0.0, "Movement Type"=0}, "Acquisition Parameters"={"Brightness"=0.0, "Contrast"=0.0, "Saturation"=0.0, "White level"=0.0}, "Background Path"=path "", "Reference Path"=path "", "XCalibration"=[], "YCalibration"=[], "ImageServer"={"IPAddress"="234.5.6.8", "Port"=58444}}, {"ID"=56.0, "Name"="*100TW M10", "DeviceID"={"Slot Connector"=32, "IP Adress"="192.168.10.34", "Port"=63420, "Type"="picodriver"}, "Detection Parameters"={"Contrast"=53, "Treshold"=53, "Max Intensity"=255, "Max Intensity%"=80, "Rx"=116, "Ry"=92, "R%"=50.0}, "Reverse"={"Reverse X"=FALSE, "Reverse Y"=TRUE}, "Target"={"X Target"=334.0, "Y Target"=206.0}, "Region of Interest"=[0, 0, 0, 0], "Correction Parameters"={"X"=100.0, "Y"=100.0, "Movement Type"=0}, "Acquisition Parameters"={"Brightness"=0.0, "Contrast"=0.0, "Saturation"=0.0, "White level"=0.0}, "Background Path"=path "", "Reference Path"=path "", "XCalibration"=[], "YCalibration"=[], "ImageServer"={"IPAddress"="234.5.6.8", "Port"=58445}}, {"ID"=57.0, "Name"="*100TW Preamp Up", "DeviceID"={"Slot Connector"=11, "IP Adress"="192.168.10.34", "Port"=63420, "Type"="picodriver"}, "Detection Parameters"={"Contrast"=0, "Treshold"=0, "Max Intensity"=0, "Max Intensity%"=0, "Rx"=0, "Ry"=0, "R%"=0.0}, "Reverse"={"Reverse X"=FALSE, "Reverse Y"=FALSE}, "Target"={"X Target"=0.0, "Y Target"=0.0}, "Region of Interest"=[0, 0, 0, 0], "Correction Parameters"={"X"=0.0, "Y"=0.0, "Movement Type"=0}, "Acquisition Parameters"={"Brightness"=0.0, "Contrast"=0.0, "Saturation"=0.0, "White level"=0.0}, "Background Path"=path "", "Reference Path"=path "", "XCalibration"=[], "YCalibration"=[], "ImageServer"={"IPAddress"="127.0.0.1", "Port"=3500}}, {"ID"=58.0, "Name"="*100TW Input Preamp2", "DeviceID"={"Slot Connector"=12, "IP Adress"="192.168.10.34", "Port"=63420, "Type"="picodriver"}, "Detection Parameters"={"Contrast"=0, "Treshold"=0, "Max Intensity"=0, "Max Intensity%"=0, "Rx"=0, "Ry"=0, "R%"=0.0}, "Reverse"={"Reverse X"=FALSE, "Reverse Y"=FALSE}, "Target"={"X Target"=0.0, "Y Target"=0.0}, "Region of Interest"=[0, 0, 0, 0], "Correction Parameters"={"X"=0.0, "Y"=0.0, "Movement Type"=0}, "Acquisition Parameters"={"Brightness"=0.0, "Contrast"=0.0, "Saturation"=0.0, "White level"=0.0}, "Background Path"=path "", "Reference Path"=path "", "XCalibration"=[], "YCalibration"=[], "ImageServer"={"IPAddress"="127.0.0.1", "Port"=3500}}, {"ID"=59.0, "Name"="*100TW Output Preamp2", "DeviceID"={"Slot Connector"=14, "IP Adress"="192.168.10.34", "Port"=63420, "Type"="picodriver"}, "Detection Parameters"={"Contrast"=0, "Treshold"=0, "Max Intensity"=0, "Max Intensity%"=0, "Rx"=0, "Ry"=0, "R%"=0.0}, "Reverse"={"Reverse X"=FALSE, "Reverse Y"=FALSE}, "Target"={"X Target"=0.0, "Y Target"=0.0}, "Region of Interest"=[0, 0, 0, 0], "Correction Parameters"={"X"=0.0, "Y"=0.0, "Movement Type"=0}, "Acquisition Parameters"={"Brightness"=0.0, "Contrast"=0.0, "Saturation"=0.0, "White level"=0.0}, "Background Path"=path "", "Reference Path"=path "", "XCalibration"=[], "YCalibration"=[], "ImageServer"={"IPAddress"="127.0.0.1", "Port"=3500}}, {"ID"=60.0, "Name"="*100TW M0", "DeviceID"={"Slot Connector"=13, "IP Adress"="192.168.10.34", "Port"=63420, "Type"="picodriver"}, "Detection Parameters"={"Contrast"=0, "Treshold"=0, "Max Intensity"=0, "Max Intensity%"=0, "Rx"=0, "Ry"=0, "R%"=0.0}, "Reverse"={"Reverse X"=FALSE, "Reverse Y"=FALSE}, "Target"={"X Target"=0.0, "Y Target"=0.0}, "Region of Interest"=[0, 0, 0, 0], "Correction Parameters"={"X"=0.0, "Y"=0.0, "Movement Type"=0}, "Acquisition Parameters"={"Brightness"=0.0, "Contrast"=0.0, "Saturation"=0.0, "White level"=0.0}, "Background Path"=path "", "Reference Path"=path "", "XCalibration"=[], "YCalibration"=[], "ImageServer"={"IPAddress"="127.0.0.1", "Port"=3500}}, {"ID"=61.0, "Name"="*100TW M2", "DeviceID"={"Slot Connector"=21, "IP Adress"="192.168.10.34", "Port"=63420, "Type"="picodriver"}, "Detection Parameters"={"Contrast"=0, "Treshold"=0, "Max Intensity"=0, "Max Intensity%"=0, "Rx"=0, "Ry"=0, "R%"=0.0}, "Reverse"={"Reverse X"=FALSE, "Reverse Y"=FALSE}, "Target"={"X Target"=0.0, "Y Target"=0.0}, "Region of Interest"=[0, 0, 0, 0], "Correction Parameters"={"X"=0.0, "Y"=0.0, "Movement Type"=0}, "Acquisition Parameters"={"Brightness"=0.0, "Contrast"=0.0, "Saturation"=0.0, "White level"=0.0}, "Background Path"=path "", "Reference Path"=path "", "XCalibration"=[], "YCalibration"=[], "ImageServer"={"IPAddress"="127.0.0.1", "Port"=3500}}, {"ID"=62.0, "Name"="*100TW M4", "DeviceID"={"Slot Connector"=22, "IP Adress"="192.168.10.34", "Port"=63420, "Type"="picodriver"}, "Detection Parameters"={"Contrast"=0, "Treshold"=0, "Max Intensity"=0, "Max Intensity%"=0, "Rx"=0, "Ry"=0, "R%"=0.0}, "Reverse"={"Reverse X"=FALSE, "Reverse Y"=FALSE}, "Target"={"X Target"=0.0, "Y Target"=0.0}, "Region of Interest"=[0, 0, 0, 0], "Correction Parameters"={"X"=0.0, "Y"=0.0, "Movement Type"=0}, "Acquisition Parameters"={"Brightness"=0.0, "Contrast"=0.0, "Saturation"=0.0, "White level"=0.0}, "Background Path"=path "", "Reference Path"=path "", "XCalibration"=[], "YCalibration"=[], "ImageServer"={"IPAddress"="127.0.0.1", "Port"=3500}}, {"ID"=63.0, "Name"="*100TW M6", "DeviceID"={"Slot Connector"=23, "IP Adress"="192.168.10.34", "Port"=63420, "Type"="picodriver"}, "Detection Parameters"={"Contrast"=0, "Treshold"=0, "Max Intensity"=0, "Max Intensity%"=0, "Rx"=0, "Ry"=0, "R%"=0.0}, "Reverse"={"Reverse X"=FALSE, "Reverse Y"=FALSE}, "Target"={"X Target"=0.0, "Y Target"=0.0}, "Region of Interest"=[0, 0, 0, 0], "Correction Parameters"={"X"=0.0, "Y"=0.0, "Movement Type"=0}, "Acquisition Parameters"={"Brightness"=0.0, "Contrast"=0.0, "Saturation"=0.0, "White level"=0.0}, "Background Path"=path "", "Reference Path"=path "", "XCalibration"=[], "YCalibration"=[], "ImageServer"={"IPAddress"="127.0.0.1", "Port"=3500}}, {"ID"=64.0, "Name"="*100TW M8", "DeviceID"={"Slot Connector"=24, "IP Adress"="192.168.10.34", "Port"=63420, "Type"="picodriver"}, "Detection Parameters"={"Contrast"=0, "Treshold"=0, "Max Intensity"=0, "Max Intensity%"=0, "Rx"=0, "Ry"=0, "R%"=0.0}, "Reverse"={"Reverse X"=FALSE, "Reverse Y"=FALSE}, "Target"={"X Target"=0.0, "Y Target"=0.0}, "Region of Interest"=[0, 0, 0, 0], "Correction Parameters"={"X"=0.0, "Y"=0.0, "Movement Type"=0}, "Acquisition Parameters"={"Brightness"=0.0, "Contrast"=0.0, "Saturation"=0.0, "White level"=0.0}, "Background Path"=path "", "Reference Path"=path "", "XCalibration"=[], "YCalibration"=[], "ImageServer"={"IPAddress"="234.5.6.8", "Port"=58450}}, {"ID"=65.0, "Name"="*100TW M13", "DeviceID"={"Slot Connector"=33, "IP Adress"="192.168.10.34", "Port"=63420, "Type"="picodriver"}, "Detection Parameters"={"Contrast"=0, "Treshold"=0, "Max Intensity"=0, "Max Intensity%"=0, "Rx"=0, "Ry"=0, "R%"=0.0}, "Reverse"={"Reverse X"=FALSE, "Reverse Y"=FALSE}, "Target"={"X Target"=0.0, "Y Target"=0.0}, "Region of Interest"=[0, 0, 0, 0], "Correction Parameters"={"X"=0.0, "Y"=0.0, "Movement Type"=0}, "Acquisition Parameters"={"Brightness"=0.0, "Contrast"=0.0, "Saturation"=0.0, "White level"=0.0}, "Background Path"=path "", "Reference Path"=path "", "XCalibration"=[], "YCalibration"=[], "ImageServer"={"IPAddress"="127.0.0.1", "Port"=3500}}, {"ID"=0.0, "Name"="*100TW M20", "DeviceID"={"Slot Connector"=1, "IP Adress"="192.168.10.184", "Port"=63430, "Type"="picodriver"}, "Detection Parameters"={"Contrast"=66, "Treshold"=66, "Max Intensity"=255, "Max Intensity%"=80, "Rx"=30, "Ry"=30, "R%"=50.0}, "Reverse"={"Reverse X"=TRUE, "Reverse Y"=TRUE}, "Target"={"X Target"=295.0, "Y Target"=162.0}, "Region of Interest"=[0, 0, 0, 0], "Correction Parameters"={"X"=20.0, "Y"=20.0, "Movement Type"=0}, "Acquisition Parameters"={"Brightness"=0.0, "Contrast"=0.0, "Saturation"=0.0, "White level"=0.0}, "Background Path"=path "", "Reference Path"=path "", "XCalibration"=[{-23000.0, -242.0}, {-22000.0, -229.0}, {-21000.0, -215.0}, {-20000.0, -203.0}, {-19000.0, -192.0}, {-18000.0, -182.0}, {-17000.0, -172.0}, {-16000.0, -162.0}, {-15000.0, -153.0}, {-14000.0, -141.0}, {-13000.0, -126.0}, {-12000.0, -105.0}, {-11000.0, -77.0}, {-10000.0, -44.0}, {0.0, 4.0}, {11000.0, 98.0}, {12000.0, 109.0}, {13000.0, 119.0}, {14000.0, 130.0}, {15000.0, 140.0}, {16000.0, 151.0}, {17000.0, 161.0}, {18000.0, 171.0}, {19000.0, 182.0}, {20000.0, 193.0}, {21000.0, 205.0}, {22000.0, 217.0}, {23000.0, 229.0}], "YCalibration"=[{-23000.0, 196.0}, {-22000.0, 189.0}, {-21000.0, 182.0}, {-20000.0, 174.0}, {-19000.0, 164.0}, {-18000.0, 153.0}, {-17000.0, 141.0}, {-16000.0, 133.0}, {-15000.0, 126.0}, {-14000.0, 117.0}, {-13000.0, 105.0}, {-12000.0, 90.0}, {-11000.0, 69.0}, {-10000.0, 42.0}, {0.0, -4.0}, {11000.0, -96.0}, {12000.0, -99.0}, {13000.0, -101.0}, {14000.0, -103.0}, {15000.0, -109.0}, {16000.0, -118.0}, {17000.0, -129.0}, {18000.0, -143.0}, {19000.0, -155.0}, {20000.0, -166.0}, {21000.0, -174.0}, {22000.0, -181.0}, {23000.0, -187.0}], "ImageServer"={"IPAddress"="234.5.6.8", "Port"=58443}}, {"ID"=12.0, "Name"="*100TW M22", "DeviceID"={"Slot Connector"=3, "IP Adress"="192.168.10.184", "Port"=63430, "Type"="picodriver"}, "Detection Parameters"={"Contrast"=59, "Treshold"=59, "Max Intensity"=255, "Max Intensity%"=80, "Rx"=47, "Ry"=33, "R%"=50.0}, "Reverse"={"Reverse X"=FALSE, "Reverse Y"=TRUE}, "Target"={"X Target"=319.0, "Y Target"=219.0}, "Region of Interest"=[0, 0, 0, 0], "Correction Parameters"={"X"=10000.0, "Y"=10000.0, "Movement Type"=0}, "Acquisition Parameters"={"Brightness"=0.0, "Contrast"=0.0, "Saturation"=0.0, "White level"=0.0}, "Background Path"=path "", "Reference Path"=path "", "XCalibration"=[], "YCalibration"=[], "ImageServer"={"IPAddress"="234.5.6.8", "Port"=58446}}, {"ID"=12.0, "Name"="*100TW M23", "DeviceID"={"Slot Connector"=4, "IP Adress"="192.168.10.184", "Port"=63430, "Type"="picodriver"}, "Detection Parameters"={"Contrast"=11, "Treshold"=11, "Max Intensity"=255, "Max Intensity%"=90, "Rx"=180, "Ry"=110, "R%"=50.0}, "Reverse"={"Reverse X"=FALSE, "Reverse Y"=TRUE}, "Target"={"X Target"=303.0, "Y Target"=342.0}, "Region of Interest"=[0, 0, 0, 0], "Correction Parameters"={"X"=0.0, "Y"=0.0, "Movement Type"=0}, "Acquisition Parameters"={"Brightness"=0.0, "Contrast"=0.0, "Saturation"=0.0, "White level"=0.0}, "Background Path"=path "", "Reference Path"=path "", "XCalibration"=[], "YCalibration"=[], "ImageServer"={"IPAddress"="234.5.6.8", "Port"=58442}}, {"ID"=6.0, "Name"="no pico", "DeviceID"={"Slot Connector"=0, "IP Adress"="127.0.0.1", "Port"=0, "Type"="picodriver"}, "Detection Parameters"={"Contrast"=0, "Treshold"=0, "Max Intensity"=0, "Max Intensity%"=0, "Rx"=0, "Ry"=0, "R%"=0.0}, "Reverse"={"Reverse X"=FALSE, "Reverse Y"=FALSE}, "Target"={"X Target"=0.0, "Y Target"=0.0}, "Region of Interest"=[0, 0, 0, 0], "Correction Parameters"={"X"=0.0, "Y"=0.0, "Movement Type"=0}, "Acquisition Parameters"={"Brightness"=0.0, "Contrast"=0.0, "Saturation"=0.0, "White level"=0.0}, "Background Path"=path "", "Reference Path"=path "", "XCalibration"=[], "YCalibration"=[], "ImageServer"={"IPAddress"="127.0.0.1", "Port"=3500}}, {"ID"=6.0, "Name"="no pico", "DeviceID"={"Slot Connector"=0, "IP Adress"="127.0.0.1", "Port"=0, "Type"="picodriver"}, "Detection Parameters"={"Contrast"=0, "Treshold"=0, "Max Intensity"=0, "Max Intensity%"=0, "Rx"=0, "Ry"=0, "R%"=0.0}, "Reverse"={"Reverse X"=FALSE, "Reverse Y"=FALSE}, "Target"={"X Target"=0.0, "Y Target"=0.0}, "Region of Interest"=[0, 0, 0, 0], "Correction Parameters"={"X"=0.0, "Y"=0.0, "Movement Type"=0}, "Acquisition Parameters"={"Brightness"=0.0, "Contrast"=0.0, "Saturation"=0.0, "White level"=0.0}, "Background Path"=path "", "Reference Path"=path "", "XCalibration"=[], "YCalibration"=[], "ImageServer"={"IPAddress"="127.0.0.1", "Port"=3500}}, {"ID"=6.0, "Name"="no pico", "DeviceID"={"Slot Connector"=0, "IP Adress"="127.0.0.1", "Port"=0, "Type"="picodriver"}, "Detection Parameters"={"Contrast"=0, "Treshold"=0, "Max Intensity"=0, "Max Intensity%"=0, "Rx"=0, "Ry"=0, "R%"=0.0}, "Reverse"={"Reverse X"=FALSE, "Reverse Y"=FALSE}, "Target"={"X Target"=0.0, "Y Target"=0.0}, "Region of Interest"=[0, 0, 0, 0], "Correction Parameters"={"X"=0.0, "Y"=0.0, "Movement Type"=0}, "Acquisition Parameters"={"Brightness"=0.0, "Contrast"=0.0, "Saturation"=0.0, "White level"=0.0}, "Background Path"=path "", "Reference Path"=path "", "XCalibration"=[], "YCalibration"=[], "ImageServer"={"IPAddress"="127.0.0.1", "Port"=3500}}, {"ID"=6.0, "Name"="mobile no ir", "DeviceID"={"Slot Connector"=0, "IP Adress"="127.0.0.1", "Port"=0, "Type"="picodriver"}, "Detection Parameters"={"Contrast"=0, "Treshold"=0, "Max Intensity"=0, "Max Intensity%"=0, "Rx"=0, "Ry"=0, "R%"=0.0}, "Reverse"={"Reverse X"=FALSE, "Reverse Y"=FALSE}, "Target"={"X Target"=0.0, "Y Target"=0.0}, "Region of Interest"=[0, 0, 0, 0], "Correction Parameters"={"X"=0.0, "Y"=0.0, "Movement Type"=0}, "Acquisition Parameters"={"Brightness"=0.0, "Contrast"=0.0, "Saturation"=0.0, "White level"=0.0}, "Background Path"=path "", "Reference Path"=path "", "XCalibration"=[], "YCalibration"=[], "ImageServer"={"IPAddress"="127.0.0.1", "Port"=3500}}, {"ID"=1.0, "Name"="regen out-salad#1", "DeviceID"={"Slot Connector"=11, "IP Adress"="192.168.10.11", "Port"=63450, "Type"="picodriver"}, "Detection Parameters"={"Contrast"=0, "Treshold"=0, "Max Intensity"=0, "Max Intensity%"=0, "Rx"=0, "Ry"=0, "R%"=0.0}, "Reverse"={"Reverse X"=FALSE, "Reverse Y"=FALSE}, "Target"={"X Target"=0.0, "Y Target"=0.0}, "Region of Interest"=[0, 0, 0, 0], "Correction Parameters"={"X"=0.0, "Y"=0.0, "Movement Type"=0}, "Acquisition Parameters"={"Brightness"=0.0, "Contrast"=0.0, "Saturation"=0.0, "White level"=0.0}, "Background Path"=path "", "Reference Path"=path "", "XCalibration"=[], "YCalibration"=[], "ImageServer"={"IPAddress"="127.0.0.1", "Port"=3500}}, {"ID"=2.0, "Name"="preamp in-salad#2", "DeviceID"={"Slot Connector"=12, "IP Adress"="192.168.10.11", "Port"=63450, "Type"="picodriver"}, "Detection Parameters"={"Contrast"=0, "Treshold"=0, "Max Intensity"=0, "Max Intensity%"=0, "Rx"=0, "Ry"=0, "R%"=0.0}, "Reverse"={"Reverse X"=FALSE, "Reverse Y"=FALSE}, "Target"={"X Target"=0.0, "Y Target"=0.0}, "Region of Interest"=[0, 0, 0, 0], "Correction Parameters"={"X"=0.0, "Y"=0.0, "Movement Type"=0}, "Acquisition Parameters"={"Brightness"=0.0, "Contrast"=0.0, "Saturation"=0.0, "White level"=0.0}, "Background Path"=path "", "Reference Path"=path "", "XCalibration"=[], "YCalibration"=[], "ImageServer"={"IPAddress"="127.0.0.1", "Port"=3500}}, {"ID"=3.0, "Name"="XPW 1", "DeviceID"={"Slot Connector"=13, "IP Adress"="192.168.10.11", "Port"=63450, "Type"="picodriver"}, "Detection Parameters"={"Contrast"=0, "Treshold"=0, "Max Intensity"=0, "Max Intensity%"=0, "Rx"=0, "Ry"=0, "R%"=0.0}, "Reverse"={"Reverse X"=FALSE, "Reverse Y"=FALSE}, "Target"={"X Target"=0.0, "Y Target"=0.0}, "Region of Interest"=[0, 0, 0, 0], "Correction Parameters"={"X"=0.0, "Y"=0.0, "Movement Type"=0}, "Acquisition Parameters"={"Brightness"=0.0, "Contrast"=0.0, "Saturation"=0.0, "White level"=0.0}, "Background Path"=path "", "Reference Path"=path "", "XCalibration"=[], "YCalibration"=[], "ImageServer"={"IPAddress"="127.0.0.1", "Port"=3500}}, {"ID"=4.0, "Name"="blue periscope regen", "DeviceID"={"Slot Connector"=14, "IP Adress"="192.168.10.11", "Port"=63450, "Type"="picodriver"}, "Detection Parameters"={"Contrast"=0, "Treshold"=0, "Max Intensity"=0, "Max Intensity%"=0, "Rx"=0, "Ry"=0, "R%"=0.0}, "Reverse"={"Reverse X"=FALSE, "Reverse Y"=FALSE}, "Target"={"X Target"=0.0, "Y Target"=0.0}, "Region of Interest"=[0, 0, 0, 0], "Correction Parameters"={"X"=0.0, "Y"=0.0, "Movement Type"=0}, "Acquisition Parameters"={"Brightness"=0.0, "Contrast"=0.0, "Saturation"=0.0, "White level"=0.0}, "Background Path"=path "", "Reference Path"=path "", "XCalibration"=[], "YCalibration"=[], "ImageServer"={"IPAddress"="127.0.0.1", "Port"=3500}}, {"ID"=8.0, "Name"="godzilla 1st", "DeviceID"={"Slot Connector"=22, "IP Adress"="192.168.10.11", "Port"=63450, "Type"="picodriver"}, "Detection Parameters"={"Contrast"=0, "Treshold"=0, "Max Intensity"=0, "Max Intensity%"=0, "Rx"=0, "Ry"=0, "R%"=0.0}, "Reverse"={"Reverse X"=FALSE, "Reverse Y"=FALSE}, "Target"={"X Target"=0.0, "Y Target"=0.0}, "Region of Interest"=[0, 0, 0, 0], "Correction Parameters"={"X"=0.0, "Y"=0.0, "Movement Type"=0}, "Acquisition Parameters"={"Brightness"=0.0, "Contrast"=0.0, "Saturation"=0.0, "White level"=0.0}, "Background Path"=path "", "Reference Path"=path "", "XCalibration"=[], "YCalibration"=[], "ImageServer"={"IPAddress"="127.0.0.1", "Port"=3500}}, {"ID"=9.0, "Name"="godzilla IN", "DeviceID"={"Slot Connector"=21, "IP Adress"="192.168.10.11", "Port"=63450, "Type"="picodriver"}, "Detection Parameters"={"Contrast"=0, "Treshold"=0, "Max Intensity"=0, "Max Intensity%"=0, "Rx"=0, "Ry"=0, "R%"=0.0}, "Reverse"={"Reverse X"=FALSE, "Reverse Y"=FALSE}, "Target"={"X Target"=0.0, "Y Target"=0.0}, "Region of Interest"=[0, 0, 0, 0], "Correction Parameters"={"X"=0.0, "Y"=0.0, "Movement Type"=0}, "Acquisition Parameters"={"Brightness"=0.0, "Contrast"=0.0, "Saturation"=0.0, "White level"=0.0}, "Background Path"=path "", "Reference Path"=path "", "XCalibration"=[], "YCalibration"=[], "ImageServer"={"IPAddress"="127.0.0.1", "Port"=3500}}, {"ID"=10.0, "Name"="Chihuahua IN", "DeviceID"={"Slot Connector"=23, "IP Adress"="192.168.10.11", "Port"=63450, "Type"="picodriver"}, "Detection Parameters"={"Contrast"=0, "Treshold"=0, "Max Intensity"=0, "Max Intensity%"=0, "Rx"=0, "Ry"=0, "R%"=0.0}, "Reverse"={"Reverse X"=FALSE, "Reverse Y"=FALSE}, "Target"={"X Target"=0.0, "Y Target"=0.0}, "Region of Interest"=[0, 0, 0, 0], "Correction Parameters"={"X"=0.0, "Y"=0.0, "Movement Type"=0}, "Acquisition Parameters"={"Brightness"=0.0, "Contrast"=0.0, "Saturation"=0.0, "White level"=0.0}, "Background Path"=path "", "Reference Path"=path "", "XCalibration"=[], "YCalibration"=[], "ImageServer"={"IPAddress"="127.0.0.1", "Port"=3500}}, {"ID"=11.0, "Name"="Chihuahua 1st", "DeviceID"={"Slot Connector"=24, "IP Adress"="192.168.10.11", "Port"=63450, "Type"="picodriver"}, "Detection Parameters"={"Contrast"=0, "Treshold"=0, "Max Intensity"=0, "Max Intensity%"=0, "Rx"=0, "Ry"=0, "R%"=0.0}, "Reverse"={"Reverse X"=FALSE, "Reverse Y"=FALSE}, "Target"={"X Target"=0.0, "Y Target"=0.0}, "Region of Interest"=[0, 0, 0, 0], "Correction Parameters"={"X"=0.0, "Y"=0.0, "Movement Type"=0}, "Acquisition Parameters"={"Brightness"=0.0, "Contrast"=0.0, "Saturation"=0.0, "White level"=0.0}, "Background Path"=path "", "Reference Path"=path "", "XCalibration"=[], "YCalibration"=[], "ImageServer"={"IPAddress"="127.0.0.1", "Port"=3500}}, {"ID"=12.0, "Name"="??XPW pico2", "DeviceID"={"Slot Connector"=34, "IP Adress"="192.168.10.11", "Port"=63450, "Type"="picodriver"}, "Detection Parameters"={"Contrast"=0, "Treshold"=0, "Max Intensity"=0, "Max Intensity%"=0, "Rx"=0, "Ry"=0, "R%"=0.0}, "Reverse"={"Reverse X"=FALSE, "Reverse Y"=FALSE}, "Target"={"X Target"=0.0, "Y Target"=0.0}, "Region of Interest"=[0, 0, 0, 0], "Correction Parameters"={"X"=0.0, "Y"=0.0, "Movement Type"=0}, "Acquisition Parameters"={"Brightness"=0.0, "Contrast"=0.0, "Saturation"=0.0, "White level"=0.0}, "Background Path"=path "", "Reference Path"=path "", "XCalibration"=[], "YCalibration"=[], "ImageServer"={"IPAddress"="127.0.0.1", "Port"=3500}}, {"ID"=13.0, "Name"="Preamp 3rd pass", "DeviceID"={"Slot Connector"=31, "IP Adress"="192.168.10.11", "Port"=63450, "Type"="picodriver"}, "Detection Parameters"={"Contrast"=0, "Treshold"=0, "Max Intensity"=0, "Max Intensity%"=0, "Rx"=0, "Ry"=0, "R%"=0.0}, "Reverse"={"Reverse X"=FALSE, "Reverse Y"=FALSE}, "Target"={"X Target"=0.0, "Y Target"=0.0}, "Region of Interest"=[0, 0, 0, 0], "Correction Parameters"={"X"=0.0, "Y"=0.0, "Movement Type"=0}, "Acquisition Parameters"={"Brightness"=0.0, "Contrast"=0.0, "Saturation"=0.0, "White level"=0.0}, "Background Path"=path "", "Reference Path"=path "", "XCalibration"=[], "YCalibration"=[], "ImageServer"={"IPAddress"="127.0.0.1", "Port"=3500}}, {"ID"=14.0, "Name"="Blue regen out", "DeviceID"={"Slot Connector"=33, "IP Adress"="192.168.10.11", "Port"=63450, "Type"="picodriver"}, "Detection Parameters"={"Contrast"=0, "Treshold"=0, "Max Intensity"=0, "Max Intensity%"=0, "Rx"=0, "Ry"=0, "R%"=0.0}, "Reverse"={"Reverse X"=FALSE, "Reverse Y"=FALSE}, "Target"={"X Target"=0.0, "Y Target"=0.0}, "Region of Interest"=[0, 0, 0, 0], "Correction Parameters"={"X"=0.0, "Y"=0.0, "Movement Type"=0}, "Acquisition Parameters"={"Brightness"=0.0, "Contrast"=0.0, "Saturation"=0.0, "White level"=0.0}, "Background Path"=path "", "Reference Path"=path "", "XCalibration"=[], "YCalibration"=[], "ImageServer"={"IPAddress"="127.0.0.1", "Port"=3500}}] {"Acquisition Parameters"."White level" scale=0.3..1.26 scale format="%#_2f"; "Acquisition Parameters"."Saturation" scale=0.5..1.5 scale format="%#_3f"; "Acquisition Parameters"."Contrast" scale=0.4..1.5 scale format="%#_3f"; "Acquisition Parameters"."Brightness" scale=-50.0..50.0 scale format="%#_2f"; "Correction Parameters"."Movement Type" items=["Step", "Proportionnal"]; "Target"."X Target" format="%#_5g"; "Target"."Y Target" format="%#_5g"; "Detection Parameters"."Max Intensity%" max=100 step=1}
  out "Images for analysis":T1[](array[typedef])=["imageserver0", "imageserver1", "imageserver2", "imageserver3", "imageserver4", "imageserver5"]
  out "history last shots":T17(array[cluster])
  out "Fancy Display":picture
  in  "Main tab":T18(tab)=enum."Expert Configure"
  out "Detection status":string[](array[string])
  out "MirrorsNames":string[](array[string])
  in  "CamOn":bool[](array[boolean])=[FALSE, FALSE, FALSE, FALSE, FALSE, FALSE, FALSE, FALSE, FALSE]
  in  "Auto":bool[](array[boolean])=[FALSE, FALSE, FALSE, FALSE, FALSE, FALSE, FALSE, FALSE, FALSE]
  out "Last Move":string[](array[string])
  out "Timeout":bool[](array[boolean])
  out "element 9":string
  out "element 8":string
  out "element 7":string
  out "element 6":string
  out "element 5":string
  out "element 4":string
  out "element 3":string
  out "element 2":string
  out "Image 9":T1(plugin-control) caption="no cam"
  out "Image 8":T1(plugin-control) caption="no cam"
  out "Image 7":T1(plugin-control) caption="no cam"
  out "Image 6":T1(plugin-control) caption="no cam"
  out "Image 5":T1(plugin-control) caption="no cam"
  out "Image 4":T1(plugin-control) caption="no cam"
  out "Image 3":T1(plugin-control) caption="no cam"
  out "Image 2":T1(plugin-control) caption="no cam"
  out "Image":T1(plugin-control) caption="TS-253a_in"
  out "element":string
  out "1":bool
  out "1 2":bool
  out "1 3":bool
  out "1 4":bool
  out "1 5":bool
  out "1 6":bool
  out "1 7":bool
  out "1 8":bool
  out "1 9":bool
  out "History Display 2":cluster{timestamp[], dbl[]}[](graph)
  in  "History # of points":i32=1000
  out "History Display 3":cluster{timestamp[], dbl[]}[](graph)
  out "History Display 4":cluster{timestamp[], dbl[]}[](graph)
  out "History Display 5":cluster{timestamp[], dbl[]}[](graph)
  out "History Display 6":cluster{timestamp[], dbl[]}[](graph)
  out "History Display 7":cluster{timestamp[], dbl[]}[](graph)
  out "History Display 8":cluster{timestamp[], dbl[]}[](graph)
  out "History Display 9":cluster{timestamp[], dbl[]}[](graph)
  out "History Display 10":cluster{timestamp[], dbl[]}[](graph)
  out "will move":bool caption="Move In Progress"
  in  "Image Selector":u16(ring) items=["Acquired Image", "Averaged Image", "Thresholded Image"]
  in  "Tab Control":T19(tab)=enum."Correction"
  in  "Tab Control 4":enum32{"User", "Advanced 1", "Advanced 2"}(tab)
  in  "Auto Detect Param":bool
  in  "Set Target (Cursor)":bool
  in  "Set Centroid as Target":bool
  in  "Target":cluster{"X Target":sgl, "Y Target":sgl}={"X Target"=334.0, "Y Target"=206.0} {"X Target" format="%#_5g"; "Y Target" format="%#_5g"}
  in  "Grab reference Image":bool
  in  "Grab Backround Image":bool
  in  "Substract":u16(ring) items=["None", "Background", "Reference"]
  in  "Reset ROI":bool
  in  "Select ROI":bool
  in  "smooth":bool=TRUE
  in  "Size & Tolerance":T20={"X Size"=5, "Y Size"=5, "% Tolerance"=10}
  out "Centroid Detection":bool=TRUE caption="Detection"
  in  "Detection Parameters":T21={"Contrast"=53, "Treshold"=53, "Max Intensity"=255, "Max Intensity%"=80, "Rx"=116, "Ry"=92, "R%"=50.0} {"Max Intensity%" max=100 step=1}
  out "Img Data":T22 caption="Current Image Data" {"Centroid"."X" format="%#_5g"; "Centroid"."Y" format="%#_5g"; "Max Intensity" format="%#_4g"; "Radius"."Rx" format="%#_5g"; "Radius"."Ry" format="%#_5g"}
  out "ImgData Avg":T23={"Centroid Avg"={"X"=334.0, "Y"=201.0}, "Max Intensity Avg"=255.0, "Radius Avg"={"Rx"=122.0, "Ry"=109.0}} caption="Data Average" {"Centroid Avg"."X" format="%#_5g"; "Centroid Avg"."Y" format="%#_5g"; "Max Intensity Avg" format="%#_4g"; "Radius Avg"."Rx" format="%#_5g"; "Radius Avg"."Ry" format="%#_5g"}
  in  "Pretreatment":bool
  in  "milliseconds to wait":u32
  in  "# imgs/trigger":i32=3 caption="# imgs grabbed after trigger"
  in  "Avg data/ data of avg img":bool
  in  "Tab Control 3":enum32{"User", "Advanced 1", "Advanced 2"}(tab)
  in  "# imgs to avg":i32=10
  in  "Initiate Correction Range":i16=3 min=0 max=100 step=1
  in  "Correction Parameters":cluster{"X":sgl, "Y":sgl, "Movement Type":u16}={"X"=100.0, "Y"=100.0, "Movement Type"=0} {"Movement Type" items=["Step", "Proportionnal"]}
  out "Move":bool
  in  "Calibrate":bool
  out "% XY State True":cluster{"X":dbl, "Y":dbl}={"X"=0.0, "Y"=100.0}
  in  "Threshold [%]":dbl=50.0
  in  "use % Out of Range":bool
  in  "use Avg Out of Range?":bool=TRUE
  out "Out of Range?":cluster{"Dev. X":bool, "Dev. Y":bool}
  out "%Out of Range":cluster{"Dev. X":bool, "Dev. Y":bool}
  in  "Auto Time Out (ms)":u32=10000
  in  "Min time between moves (s)":u32=5
  in  "Mirrors":u8[](array[ring])=[50, 41, 42, 52, 53, 54] items=["no-device", "GasJet", "Godzilla_M1", "Godzilla_M2", "Godzilla_M3", "Godzilla_M4", "Godzilla_M6", "Godzilla_M8_Steer", "Chihuahua_M1", "Chihuahua_M2", "Collider_M4", "Collider_M5", "Collider_M8 Translation s3c4", "HeaterBlue-M1", "HeaterBlue-M2", "HeaterBlue-M3", "THz OAP Down", "G Spot Camera", "G Spot Monitor", "C Spot Monitor", "p15c4-Free", "THz_M5", "THz_M7A & Xtal", "THz_M7B", "THz MIrror Top", "THz OAP Top", "p2s2c2-Free", "p2s2c3-Free", "p2s2c4-Free", "Heater_M0", "Heater_M4", "Heater_M5", "Ignitor Iris", "Ignitor_M4", "Collider_M6", "Collder_M7", "C Spot Camera", "p2s5c1-FREE", "p2s5c2-FREE", "p2s5c3-FREE", "p2c5c4-FREE", "*100TW M9 - L8_M10Leak", "*100TW M10 - B1_TelInput", "Preamp Up - PA2_Input1", "*100TW Input Preamp2 - PA2_Input2", "*100TW Output Preamp2 - L1_TelInpNear", "*100TW M0 - L2_TelInpFar", "*100TW M2", "*100TW M4", "*100TW M6", "*100TW M8 - L7_TREXPass4", "*100TW M13 - B2_TelLens1", "*100TW M14 - B4_TelOutput", "*100TW M14 - B3_TelLens2", "*100TW M20 - B6_SwitchYNear", "*100TW M20 - B7_SwitchYFar", "*100TW M22 - B9_OAPFront", "*100TW M22 - B8_OAPBack", "*100TW M22 - TargetCam", "*100TW (Cam Only) - B5_CompressorOut", "*100TW (Cam Only) - PA2_Input2", "*100TW (Cam Only) - L3_TelescopeOut", "TS-253a_in", "Telescope in", "Periscope", "Chamber_In", "*100TW Main Amp 2 - L4_TREXPass1", "*100TW Main Amp 4 - L5_TREXPass2", "*100TW Main Amp 6 - L6_TREXPass3", "*100TW (Cam Only) - XtalNorth", "*100TW (Cam Only) - XtalSouth", "*100TW Main Amp 8 - BKM", "*100TW M23 - PaperCam", "*100TW M23 - Phasics", "*100TW (Cam Only) - FWMI", "*100TW (Cam Only) - Wedge", "*100TW (Cam Only) - CapSideView", "*100TW TA6", "no pico", "no pico", "no pico", "mobile no ir", "regen out-salad#1", "preamp in-salad#2", "XPW 1", "blue periscope regen", "godzilla 1st", "godzilla IN", "Chihuahua IN", "Chihuahua 1st", "??XPW pico2", "Preamp 3rd pass", "Blue regen out"]
  in  "UDP timeout ms":i32=200
  out "#loops waiting for new image":i32
  out "# loops waiting 4 move":i32
  in  "Reverse":cluster{"Reverse X":bool, "Reverse Y":bool}={"Reverse X"=FALSE, "Reverse Y"=TRUE}
  in  "Fancy Display Options":T24
  in  "Target Area  Display":T25={"Show Variance"=FALSE, "Show Target Reached"=TRUE, "Show Init Correction"=TRUE}
  in  "Display":T26={"Show Best Rect"=TRUE, "Show Centroid"=TRUE, "Show Avg Centroid"=FALSE, "Show Target"=FALSE, "Show Target Area"=TRUE}
  in  "Open CamCenter":bool
  in  "Set Color Map":bool
  in  "Acquisition Parameters":T27 {"White level" scale=0.3..1.26 scale format="%#_2f"; "Saturation" scale=0.5..1.5 scale format="%#_3f"; "Contrast" scale=0.4..1.5 scale format="%#_3f"; "Brightness" scale=-50.0..50.0 scale format="%#_2f"}
  in  "Graph":T28(tab)=enum."X Cal"
  out "X Intensity":u8[](graph)
  out "Y Intensity":u8[][](graph)
  out "Target Area":cluster{dbl[], dbl[]}[](graph)=[{[0.0, 0.0006342391823892943, 0.0012659245074418742, 0.0018925124013031524, 0.002511479815674843, 0.0031203343872399612, 0.0037166244735302428, 0.004297949024825067, 0.004861967252331248, 0.005406408053713336, 0.005929079158021155, 0.006427875953191165, 0.0069007899605764405, 0.00734591692238129, 0.0077614644694353144, 0.008145759338431443, 0.008497254109566709, 0.00881453343745564, 0.009096319750226588, 0.00934147839385275, 0.009549022201003456, 0.009718115466018603, 0.009848077310000394, 0.009938384422472335, 0.009988673168565831, 0.009998741053249468, 0.009968547536705018, 0.009898214197566995, 0.009788024243368392, 0.009638421370163911, 0.009450007975922542, 0.009223542734883563, 0.008959937542643143, 0.008660253844272625, 0.00832569836025385, 0.007957618227441692, 0.007557495574619389, 0.00712694155448907, 0.006667689856128432, 0.0061815897240367545, 0.005670598511879952, 0.005136773800918219, 0.004582265114852496, 0.004009305264451178, 0.0034202013568092296, 0.0028173255054421632, 0.0022031052786221665, 0.0015800139244174349, 0.0009505604117951475, 0.0003172793278889308, -0.00031727932788892837, -0.000950560411795145, -0.0015800139244174323, -0.0022031052786221643, -0.00281732550544216, -0.0034202013568092274, -0.004009305264451176, -0.004582265114852494, -0.005136773800918217, -0.00567059851187995, -0.006181589724036752, -0.0066676898561284295, -0.007126941554489069, -0.0075574955746193885, -0.007957618227441688, -0.008325698360253849, -0.008660253844272622, -0.008959937542643145, -0.009223542734883563, -0.00945000797592254, -0.00963842137016391, -0.009788024243368392, -0.009898214197566995, -0.009968547536705017, -0.009998741053249468, -0.009988673168565831, -0.009938384422472335, -0.009848077310000395, -0.009718115466018607, -0.009549022201003456, -0.00934147839385275, -0.009096319750226591, -0.00881453343745564, -0.008497254109566709, -0.008145759338431445, -0.007761464469435318, -0.00734591692238129, -0.006900789960576441, -0.006427875953191169, -0.00592907915802116, -0.005406408053713335, -0.004861967252331249, -0.0042979490248250705, -0.0037166244735302484, -0.0031203343872399604, -0.002511479815674844, -0.0018925124013031568, -0.001265924507441881, -0.0006342391823892944, -2.4492126529005845e-18], [0.009999999776482582, 0.00997986654165144, 0.009919547906588775, 0.009819286753148901, 0.009679486797610168, 0.009500710965052011, 0.009283679122654322, 0.009029265181046405, 0.008738493575377293, 0.008412535140276995, 0.008052702395318658, 0.007660444259965505, 0.0072373402192835385, 0.00678509396391265, 0.006305526529905721, 0.005800568966059159, 0.005272254558260948, 0.004722710642166016, 0.004154150037166373, 0.0035688621361484323, 0.0029692036869158737, 0.0023575893023980443, 0.0017364817378559118, 0.0011083819742358427, 0.0004758191476020371, -0.0001586596348017588, -0.0007924995508541375, -0.0014231483509230048, -0.0020480666348740477, -0.0026647380773388092, -0.00327067956006883, -0.003863451170576422, -0.004440666026801119, -0.0049999998882412884, -0.0055392005148503206, -0.006056096736012351, -0.00654860719308007, -0.007014748720271355, -0.007452644330177961, -0.007860530771731315, -0.008236765630192265, -0.008579833940575534, -0.008888354287879029, -0.0091610843695545, -0.009396925997821414, -0.009594929521681582, -0.009754297650828523, -0.009874388666054152, -0.009954719003225532, -0.009994965200426965, -0.009994965200426965, -0.009954719003225532, -0.009874388666054154, -0.009754297650828523, -0.009594929521681584, -0.009396925997821416, -0.0091610843695545, -0.00888835428787903, -0.008579833940575534, -0.008236765630192265, -0.007860530771731315, -0.007452644330177963, -0.007014748720271357, -0.006548607193080072, -0.006056096736012352, -0.005539200514850322, -0.004999999888241295, -0.004440666026801117, -0.003863451170576422, -0.0032706795600688323, -0.002664738077338816, -0.0020480666348740477, -0.0014231483509230072, -0.0007924995508541421, -0.0001586596348017657, 0.00047581914760203687, 0.0011083819742358403, 0.0017364817378559075, 0.002357589302398038, 0.0029692036869158737, 0.00356886213614843, 0.0041541500371663695, 0.004722710642166017, 0.005272254558260948, 0.005800568966059157, 0.006305526529905717, 0.006785093963912651, 0.007237340219283538, 0.007660444259965502, 0.008052702395318655, 0.008412535140276995, 0.008738493575377293, 0.009029265181046402, 0.00928367912265432, 0.009500710965052011, 0.009679486797610168, 0.0098192867531489, 0.009919547906588774, 0.00997986654165144, 0.009999999776482582]}, {[], []}, {[nan, nan, nan, nan, nan, nan, nan, nan, nan, nan, nan, nan, nan, nan, nan, nan, nan, nan, nan, nan, nan, nan, nan, nan, nan, nan, nan, nan, nan, nan, nan, nan, nan, nan, nan, nan, nan, nan, nan, nan, nan, nan, nan, nan, nan, nan, nan, nan, nan, nan, nan, nan, nan, nan, nan, nan, nan, nan, nan, nan, nan, nan, nan, nan, nan, nan, nan, nan, nan, nan, nan, nan, nan, nan, nan, nan, nan, nan, nan, nan, nan, nan, nan, nan, nan, nan, nan, nan, nan, nan, nan, nan, nan, nan, nan, nan, nan, nan, nan, nan], [nan, nan, nan, nan, nan, nan, nan, nan, nan, nan, nan, nan, nan, nan, nan, nan, nan, nan, nan, nan, nan, nan, nan, nan, nan, nan, nan, nan, nan, nan, nan, nan, nan, nan, nan, nan, nan, nan, nan, nan, nan, nan, nan, nan, nan, nan, nan, nan, nan, nan, nan, nan, nan, nan, nan, nan, nan, nan, nan, nan, nan, nan, nan, nan, nan, nan, nan, nan, nan, nan, nan, nan, nan, nan, nan, nan, nan, nan, nan, nan, nan, nan, nan, nan, nan, nan, nan, nan, nan, nan, nan, nan, nan, nan, nan, nan, nan, nan, nan, nan]}]
  out "History Display":T17(graph)=[{"seconds since 1Jan1904"=timestamp(3366343832.03125 s since 1904-01-01), "number: 0 to 1"=334.0, "number: 0 to 1"=201.0}, {"seconds since 1Jan1904"=timestamp(3366343831.828125 s since 1904-01-01), "number: 0 to 1"=334.0, "number: 0 to 1"=201.0}, {"seconds since 1Jan1904"=timestamp(3366343831.71875 s since 1904-01-01), "number: 0 to 1"=334.0, "number: 0 to 1"=201.0}, {"seconds since 1Jan1904"=timestamp(3366343831.59375 s since 1904-01-01), "number: 0 to 1"=334.0, "number: 0 to 1"=201.0}, {"seconds since 1Jan1904"=timestamp(3366343831.484375 s since 1904-01-01), "number: 0 to 1"=334.0, "number: 0 to 1"=201.0}, {"seconds since 1Jan1904"=timestamp(3366343831.359375 s since 1904-01-01), "number: 0 to 1"=334.0, "number: 0 to 1"=201.0}, {"seconds since 1Jan1904"=timestamp(3366343831.21875 s since 1904-01-01), "number: 0 to 1"=334.0, "number: 0 to 1"=201.0}, {"seconds since 1Jan1904"=timestamp(3366343831.09375 s since 1904-01-01), "number: 0 to 1"=334.0, "number: 0 to 1"=201.0}, {"seconds since 1Jan1904"=timestamp(3366343830.984375 s since 1904-01-01), "number: 0 to 1"=334.0, "number: 0 to 1"=201.0}, {"seconds since 1Jan1904"=timestamp(3366343830.859375 s since 1904-01-01), "number: 0 to 1"=334.0, "number: 0 to 1"=201.0}, {"seconds since 1Jan1904"=timestamp(3366343830.734375 s since 1904-01-01), "number: 0 to 1"=334.0, "number: 0 to 1"=201.0}, {"seconds since 1Jan1904"=timestamp(3366343830.59375 s since 1904-01-01), "number: 0 to 1"=334.0, "number: 0 to 1"=201.0}, {"seconds since 1Jan1904"=timestamp(3366343830.46875 s since 1904-01-01), "number: 0 to 1"=334.0, "number: 0 to 1"=201.0}, {"seconds since 1Jan1904"=timestamp(3366343830.359375 s since 1904-01-01), "number: 0 to 1"=334.0, "number: 0 to 1"=201.0}, {"seconds since 1Jan1904"=timestamp(3366343830.234375 s since 1904-01-01), "number: 0 to 1"=334.0, "number: 0 to 1"=201.0}, {"seconds since 1Jan1904"=timestamp(3366343830.109375 s since 1904-01-01), "number: 0 to 1"=334.0, "number: 0 to 1"=201.0}, {"seconds since 1Jan1904"=timestamp(3366343829.96875 s since 1904-01-01), "number: 0 to 1"=334.0, "number: 0 to 1"=201.0}, {"seconds since 1Jan1904"=timestamp(3366343829.859375 s since 1904-01-01), "number: 0 to 1"=334.0, "number: 0 to 1"=201.0}, {"seconds since 1Jan1904"=timestamp(3366343829.734375 s since 1904-01-01), "number: 0 to 1"=334.0, "number: 0 to 1"=201.0}, {"seconds since 1Jan1904"=timestamp(3366343829.578125 s since 1904-01-01), "number: 0 to 1"=334.0, "number: 0 to 1"=201.0}]
  out "X calibration":cluster{dbl, dbl}[](graph)
  out "Y calibration":cluster{dbl, dbl}[](graph)
  out "Displayed Image":u8[][](graph)
  in  "restart":bool
  out "conn req":bool caption="Move In Progress"
  out "MoveInProgress 2":bool caption="Move In Progress"
  out "Image IP":string
  out "Image to save":u8[][](graph)
  in  "ONTRAK Com Port":refnum<visa-resource-name>="COM1"
  in  "Save Changes?":bool=TRUE
  out "Warning !":string="Warning : The beam has not been detected, so the averaged and tresholded images have not been calculated"
  in  "stop":bool
  out "USB cameras Indic":i32(listbox)=1 caption="USB cameras"
  # "Beam Pointing 20120418, LOASIS Program"
  # "Times"
  # "MOTOR/CAMERA LIST"
  # "CONTROLS"
  # "INDICATORS"
  # "loop mode diagnostics"
  # "px"
  # "px"
  # "Int"
  # "Int"
  # "Int"
  # "% of Max"
  # "px"
  # "px"
  # "% of Radius"
  # "Int"
  # "Int"
  # "% of Radius"
  # "Detection settings :                                                                                                                                                                         - contrast : This parameter is used during the edge detection of the beam. Contrast specifies the threshold for the contrast of the edge. Only edges with a contrast greater than this value are used in the detection process. Contrast is defined as the difference between the average pixel intensity before the edge and the average pixel intensity after the edge.                                                                                                                                                                                     - The treshold value is used during the processing of the tresholded image. Each pixel intensity value (ranged between 0 and 255) below this parameter will be set to 0, and each pixel above this value will be set to 255.                                                     - Max intensity is maximum intensity of the beam.                                                                                                                         - Max Intensity % is the tolerance about the beam maximum intensity. Practically, to be detected, the peak intensity in the picture must be ranged between Max intensity +/- Max intensity %                                                                                             - Rx is the beam radius on the X axis (in pixels).                                                                                                                                             - Ry is the beam radius on the Y axis (in pixels).                                                                                                                                             - R% is the tolerance about the beam radius. Practically, the X and Y radius must respectively be comprised between Rx +/- R% and Ry +/- R%"
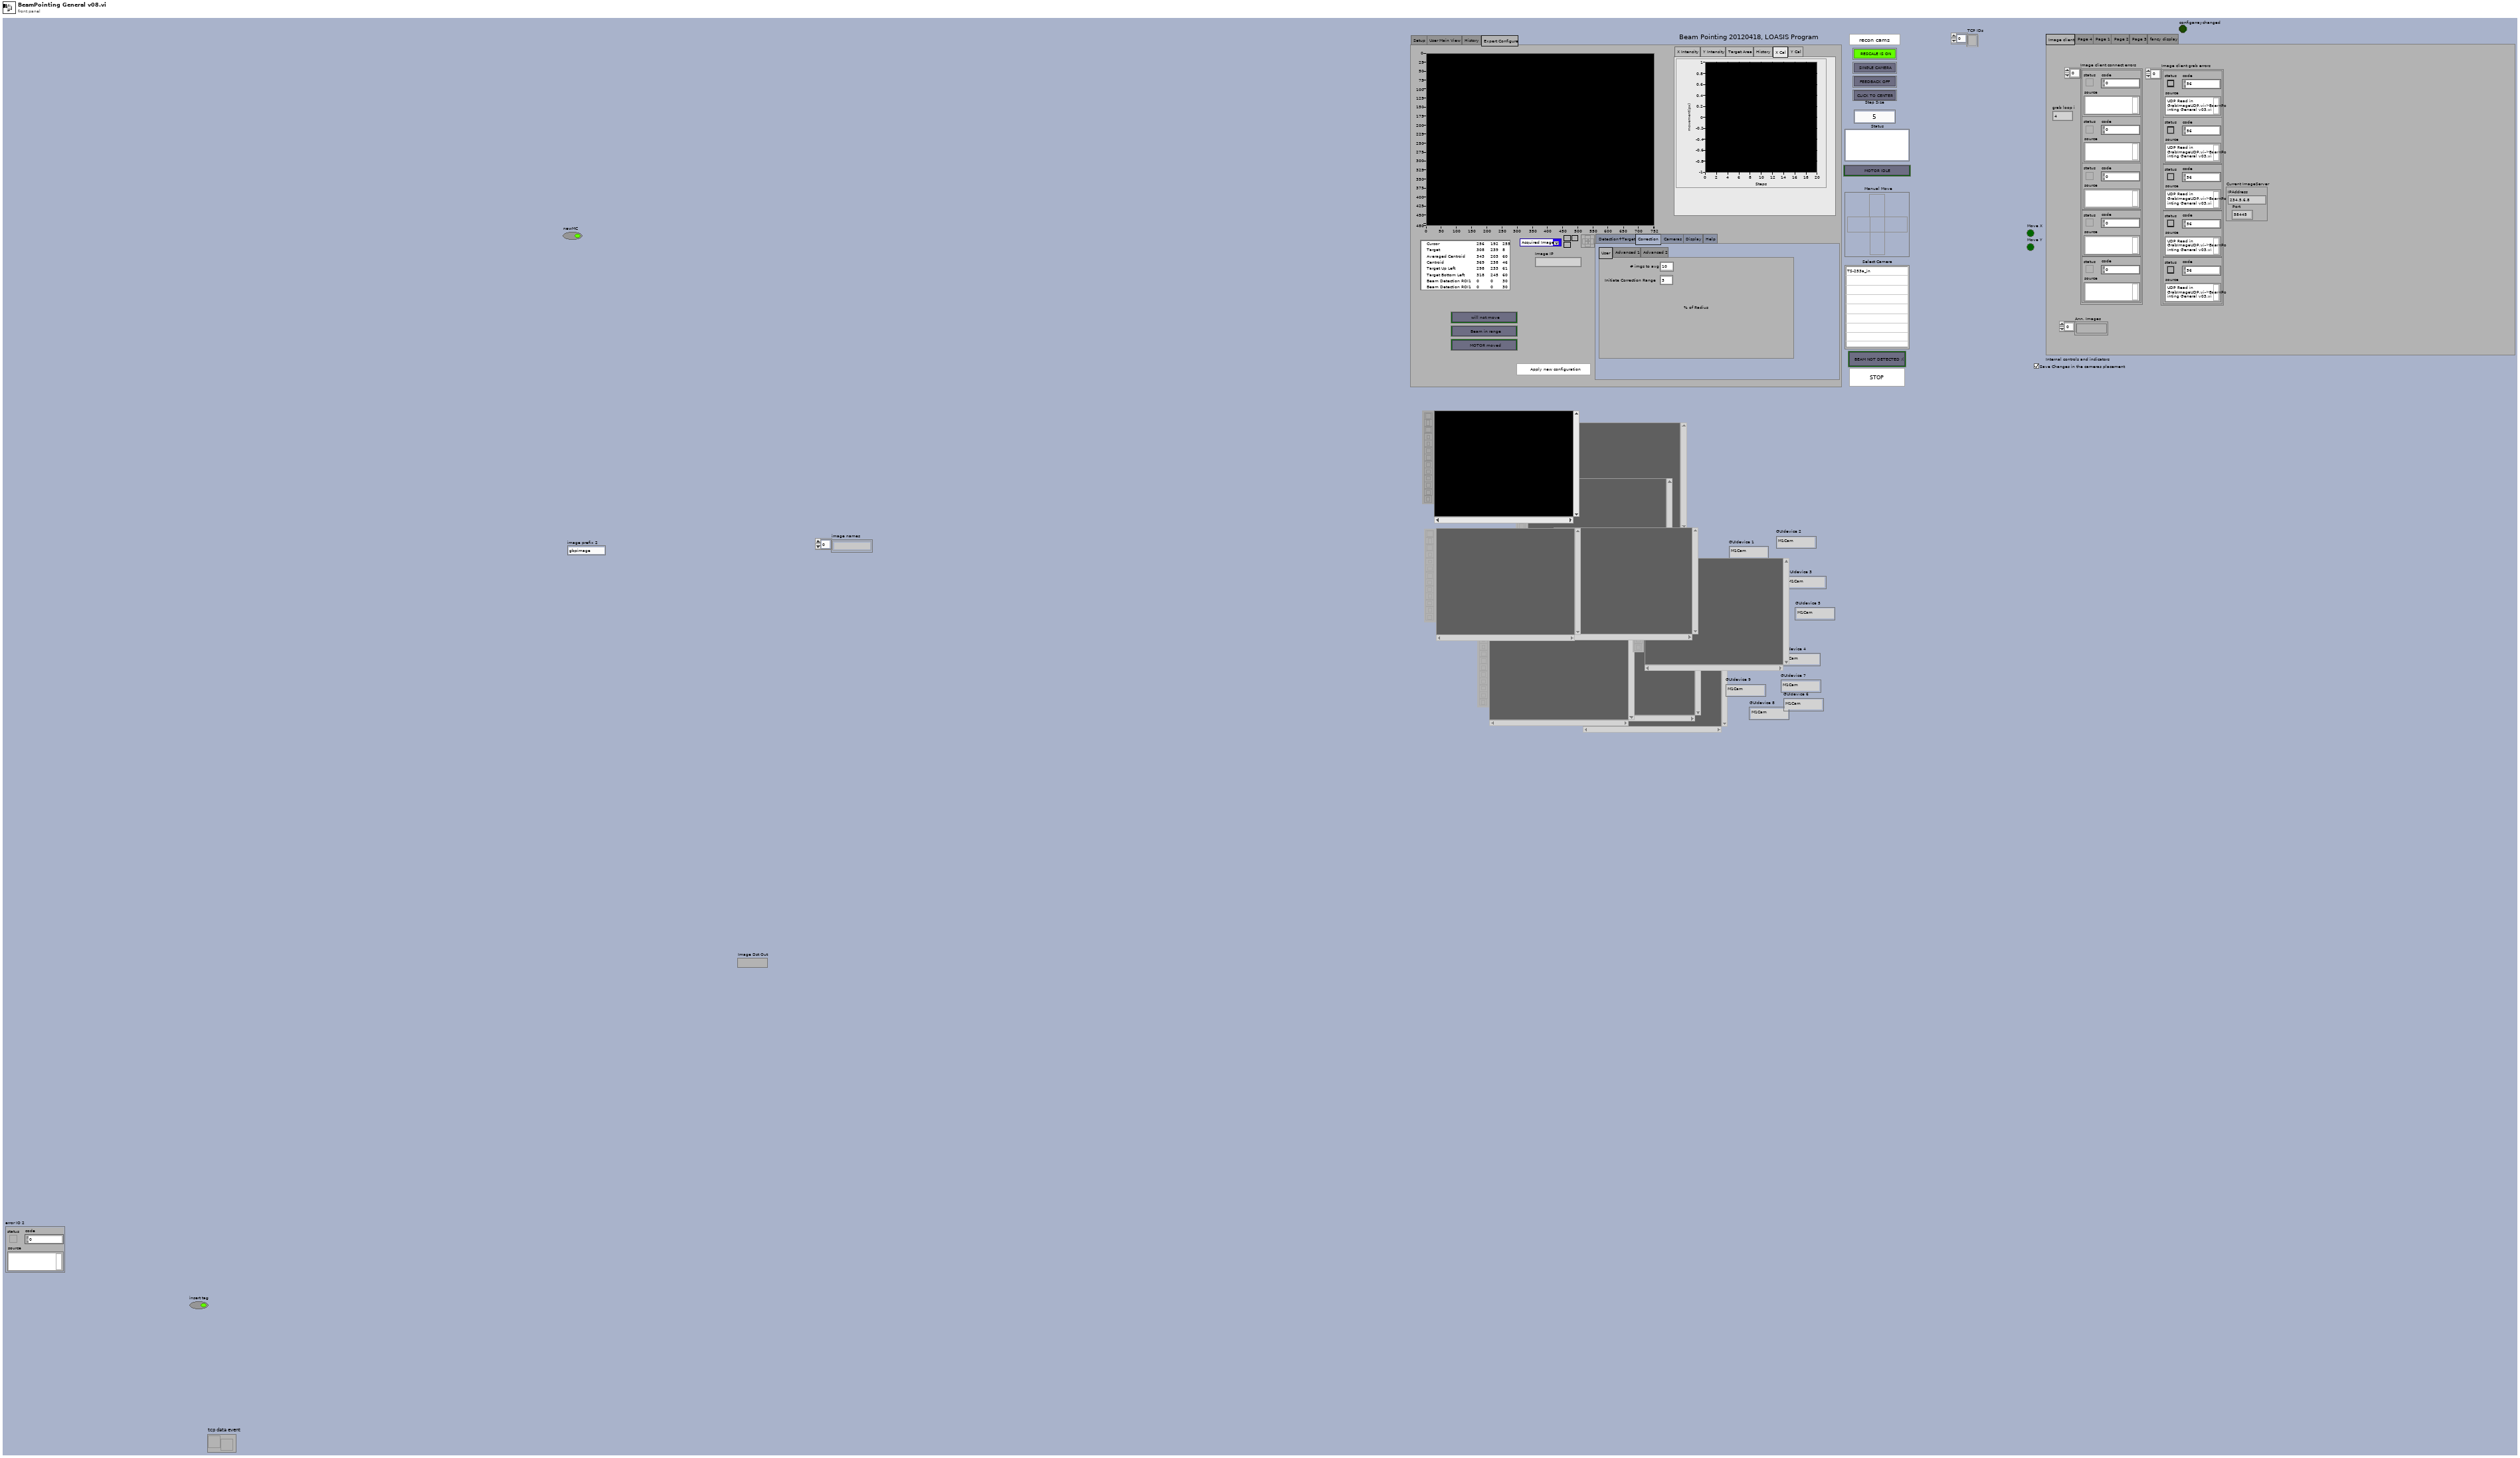
[diagram p1: front panel]
types:
  T1 = typedef "IMAQ Image.ctl" = refnum<image>
  T2 = typedef "tcp_new_data_event.ctl" = refnum<user-event>
  T3 = cluster{"Down":bool, "Up":bool, "Right":bool, "Left":bool, "APulses X":u16, "APulses Y":u16, "StopButton":bool}
  T4 = enum32{"Image client", "Page 4", "Page 1", "Page 2", "Page 3", "fancy display"}
  T5 = cluster{"Down":bool, "Up":bool, "Right":bool, "Left":bool, "APulses X":u16, "APulses Y":u16, "StopButton":bool}[]
  T6 = typedef "IMAQdx.ctl" = refnum<k21>
  T7 = cluster{"IPaddress":string, "Port":i32, "connection ID":refnum<k5>, "TCP error":errorcluster}[]
  T8 = cluster{"Add?":bool, "Channel":i32, "Device Name":string}
  T9 = cluster{"ID":dbl, "Name":string, "DeviceID":cluster{"Slot Connector":i32, "IP Adress":string, "Port":i32, "Type":string}, "CorrectConfig Cluster":cluster{"Detection Parameters":cluster{"Contrast":i32, "Treshold":u8, "Max Intensity":i32, "Max Intensity%":u8, "Rx":i32, "Ry":i32, "R%":sgl}, "Reverse":cluster{"Reverse X":bool, "Reverse Y":bool}, "Target":cluster{"X Target":sgl, "Y Target":sgl}, "Region of Interest":i32[], "Correction Parameters":cluster{"X":sgl, "Y":sgl, "Movement Type":u16}, "Acquisition Parameters":cluster{"Brightness":dbl, "Contrast":dbl, "Saturation":dbl, "White level":dbl}, "Background Path":path, "Reference Path":path, "XCalibration":cluster{dbl, dbl}[], "YCalibration":cluster{dbl, dbl}[]}, "Ontrak Channel":i16, "IMAQdx Session 2":T6, "ImageServer":cluster{"IPAddress":string, "Port":i32}}[]
  T10 = cluster{"Center":cluster{"X":sgl, "Y":sgl}, "Major Axis":cluster{"Point 1":cluster{"X":sgl, "Y":sgl}, "Point 2":cluster{"X":sgl, "Y":sgl}}, "Minor Axis":cluster{"Point 1":cluster{"X":sgl, "Y":sgl}, "Point 2":cluster{"X":sgl, "Y":sgl}}}
  T11 = cluster{"Parameter1":i32, "Parameter2":dbl, "Parameter3":dbl, "Parameter4":dbl}
  T12 = cluster{"PreviousCenter":cluster{"X":dbl, "Y":dbl}, "CurrentCenter":cluster{"X":dbl, "Y":dbl}}
  T13 = typedef "IMAQ Rectangle" = cluster{"Left":i32, "Top":i32, "Right":i32, "Bottom":i32, "Rotation":dbl}
  T14 = cluster{"seconds since 1Jan1904":timestamp, "number: 0 to 1":dbl, "number: 0 to 1":dbl}[][]
  T15 = cluster{"X Intensity":u8[], "Y Intensity":u8[], "Max Intensity":sgl, "Center":cluster{"X":sgl, "Y":sgl}, "Radius":cluster{"Rx":sgl, "Ry":sgl}}[]
  T16 = cluster{"ID":dbl, "Name":string, "DeviceID":cluster{"Slot Connector":i32, "IP Adress":string, "Port":i32, "Type":string}, "Detection Parameters":cluster{"Contrast":i32, "Treshold":u8, "Max Intensity":i32, "Max Intensity%":u8, "Rx":i32, "Ry":i32, "R%":sgl}, "Reverse":cluster{"Reverse X":bool, "Reverse Y":bool}, "Target":cluster{"X Target":sgl, "Y Target":sgl}, "Region of Interest":i32[], "Correction Parameters":cluster{"X":sgl, "Y":sgl, "Movement Type":u16}, "Acquisition Parameters":cluster{"Brightness":dbl, "Contrast":dbl, "Saturation":dbl, "White level":dbl}, "Background Path":path, "Reference Path":path, "XCalibration":cluster{dbl, dbl}[], "YCalibration":cluster{dbl, dbl}[], "ImageServer":cluster{"IPAddress":string, "Port":i32}}[]
  T17 = cluster{"seconds since 1Jan1904":timestamp, "number: 0 to 1":dbl, "number: 0 to 1":dbl}[]
  T18 = enum32{"Setup", "User Main View", "History", "Expert Configure"}
  T19 = enum32{"Detection+Target", "Correction", "Cameras", "Display", "Help"}
  T20 = cluster{"X Size":i32, "Y Size":i32, "% Tolerance":i32}
  T21 = cluster{"Contrast":i32, "Treshold":u8, "Max Intensity":i32, "Max Intensity%":u8, "Rx":i32, "Ry":i32, "R%":sgl}
  T22 = cluster{"Centroid":cluster{"X":sgl, "Y":sgl}, "Max Intensity":sgl, "Radius":cluster{"Rx":sgl, "Ry":sgl}}
  T23 = cluster{"Centroid Avg":cluster{"X":sgl, "Y":sgl}, "Max Intensity Avg":sgl, "Radius Avg":cluster{"Rx":sgl, "Ry":sgl}}
  T24 = cluster{"Use fancy display":bool, "Show Edges":bool, "Show Full Ellipse":bool, "Show Ellipses points":bool, "show acquired image":bool}
  T25 = cluster{"Show Variance":bool, "Show Target Reached":bool, "Show Init Correction":bool}
  T26 = cluster{"Show Best Rect":bool, "Show Centroid":bool, "Show Avg Centroid":bool, "Show Target":bool, "Show Target Area":bool}
  T27 = cluster{"Brightness":dbl, "Contrast":dbl, "Saturation":dbl, "White level":dbl}
  T28 = enum32{"X Intensity", "Y Intensity", "Target Area", "History", "X Cal", "Y Cal"}
  T29 = enum16{"open", "replace", "create", "open or create", "replace or create", "replace or create with confirmation"}
  T30 = cluster{"X Intensity":u8[], "Y Intensity":u8[], "Max Intensity":i32, "Center":cluster{"X":i32, "Y":i32}, "Radius":cluster{"Rx":i32, "Ry":i32}}
  T31 = cluster{"Slot Connector":i32, "IP Adress":string, "Port":i32, "Type":string}
  T32 = cluster{"left":i16, "top":i16, "right":i16, "bottom":i16}
  T33 = cluster{"Width":i16, "Style":enum32{"Solid", "Dash", "Dot", "DashDot", "DashDotDot"}}
  T34 = cluster{"Width":u16, "Style":enum32{"Solid", "Dash", "Dot", "DashDot", "DashDotDot"}}
  T35 = typedef "Image Type" = u32
  T36 = cluster{"ID":dbl, "Name":string, "DeviceID":cluster{"Slot Connector":i32, "IP Adress":string, "Port":i32, "Type":string}, "CorrectConfig Cluster":cluster{"Detection Parameters":cluster{"Contrast":i32, "Treshold":u8, "Max Intensity":i32, "Max Intensity%":u8, "Rx":i32, "Ry":i32, "R%":sgl}, "Reverse":cluster{"Reverse X":bool, "Reverse Y":bool}, "Target":cluster{"X Target":sgl, "Y Target":sgl}, "Region of Interest":i32[], "Correction Parameters":cluster{"X":sgl, "Y":sgl, "Movement Type":u16}, "Acquisition Parameters":cluster{"Brightness":dbl, "Contrast":dbl, "Saturation":dbl, "White level":dbl}, "Background Path":path, "Reference Path":path, "XCalibration":cluster{dbl, dbl}[], "YCalibration":cluster{dbl, dbl}[]}, "Ontrak Channel":i16, "IMAQdx Session 2":T6, "ImageServer":cluster{"IPAddress":string, "Port":i32}}
  T37 = cluster{"X Intensity":u8[], "Y Intensity":u8[], "Max Intensity":i32, "Center":cluster{"X":i32, "Y":i32}, "Radius":cluster{"Rx":i32, "Ry":i32}}[]
  T38 = cluster{"Down":bool, "Up":bool, "Right":bool, "Left":bool, "APulses X":i32, "APulses Y":i32, "Stop":bool}
  T39 = cluster{"Down":bool, "Up":bool, "Right":bool, "Left":bool, "APulses X":i32, "APulses Y":i32, "Stop":bool}[]
  T40 = typedef "LVPointDoubleTypeDef.ctl" = cluster{"Cursor X":dbl, "Cursor Y":dbl}
  T41 = cluster{"Show Best Rect":bool, "Show Centroid":bool}
  T42 = cluster{"X Intensity":u8[], "Y Intensity":u8[], "Max Intensity":u8, "Centroid":cluster{"X":i32, "Y":i32}, "Radius":cluster{"Rx":i32, "Ry":i32}}
  T43 = cluster{"X Intensity":u8[], "Y Intensity":u8[], "Max Intensity":sgl, "Center":cluster{"X":sgl, "Y":sgl}, "Radius":cluster{"Rx":sgl, "Ry":sgl}}
  T44 = typedef "imagedata.ctl" = cluster{"image type":i32, "image depth":i32, "image":u8[], "mask":u8[], "colors":u32[], "Rectangle":cluster{"left":i16, "top":i16, "right":i16, "bottom":i16}}
  T45 = cluster{"Left":i32, "Top":i32, "Right":i32, "Bottom":i32}
  T46 = typedef "tcp new data cluster.ctl" = cluster{"EventEnum":enum16{"new data", "connection status update"}, "Device name":string}
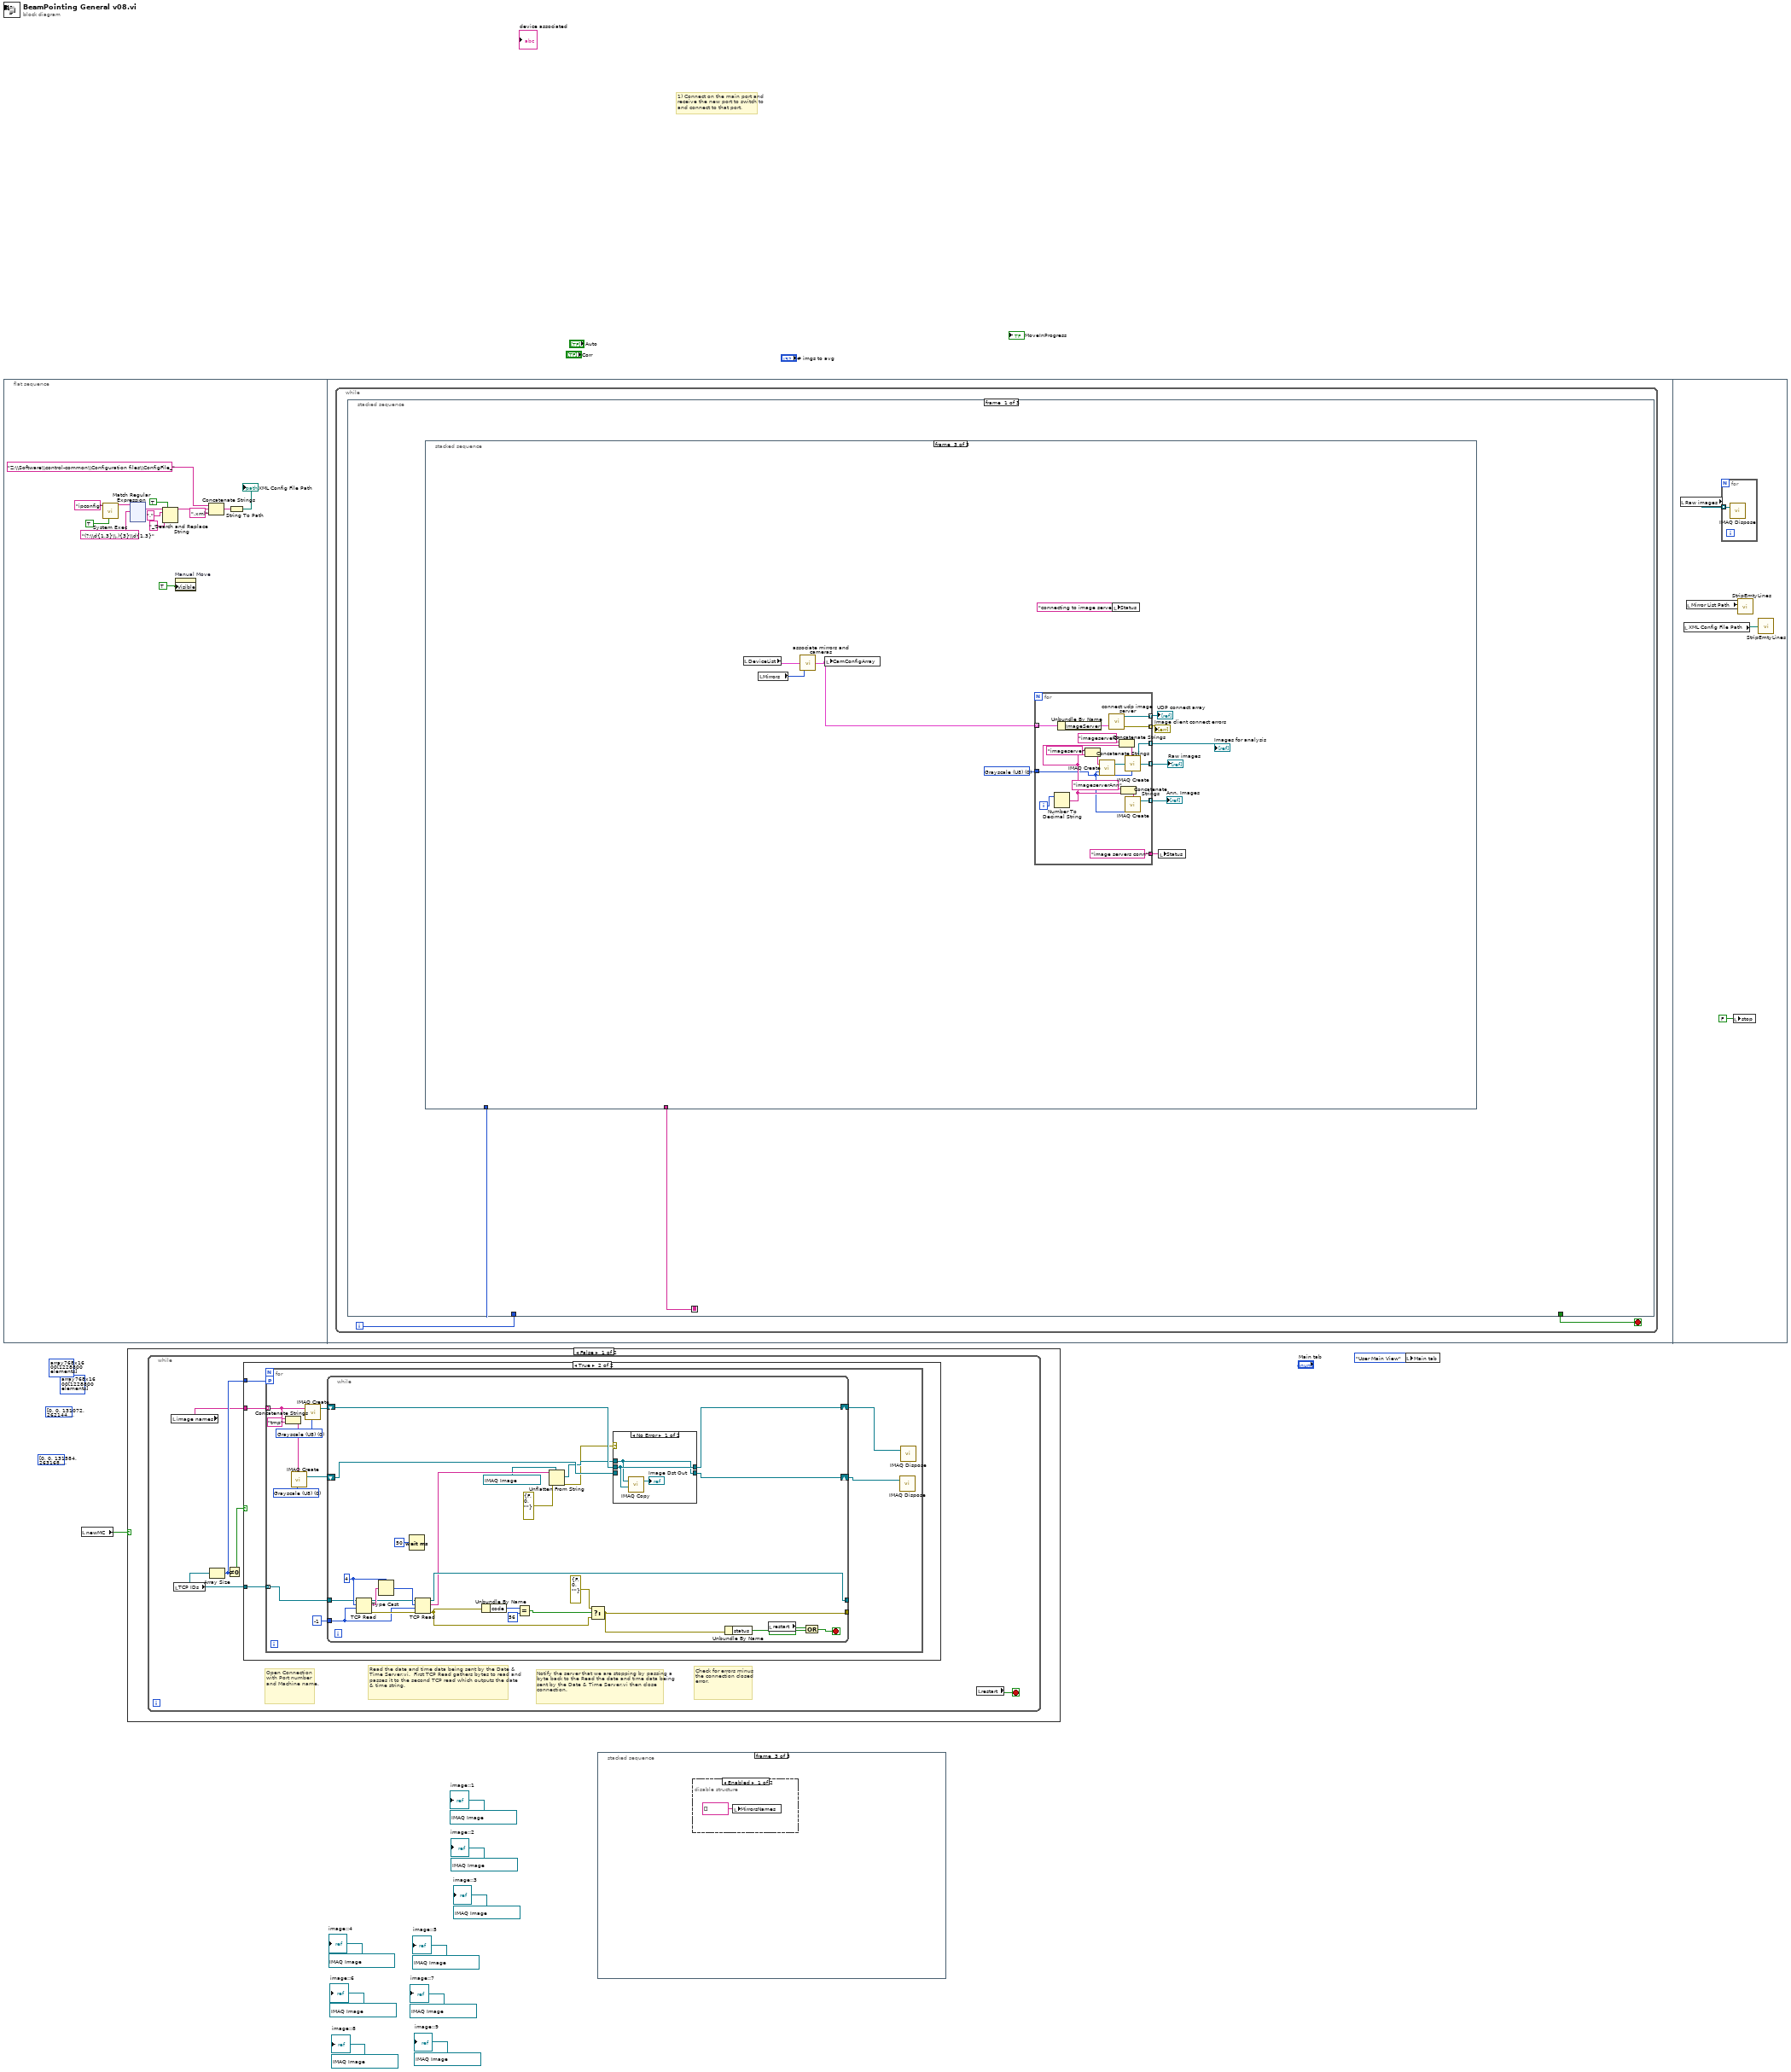
[diagram p0: block diagram]
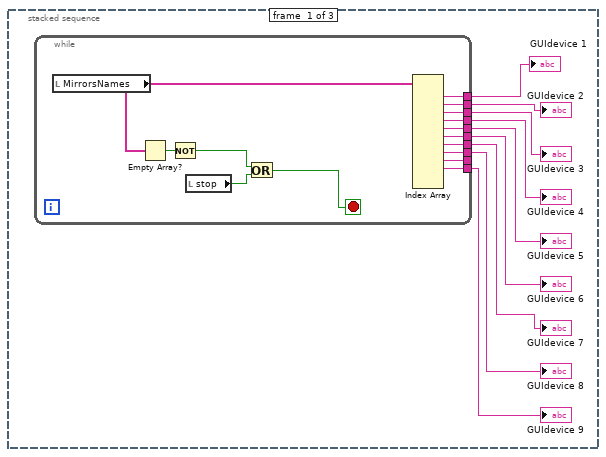
[diagram p2: hidden frame]
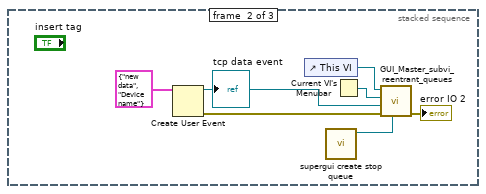
[diagram p3: hidden frame]
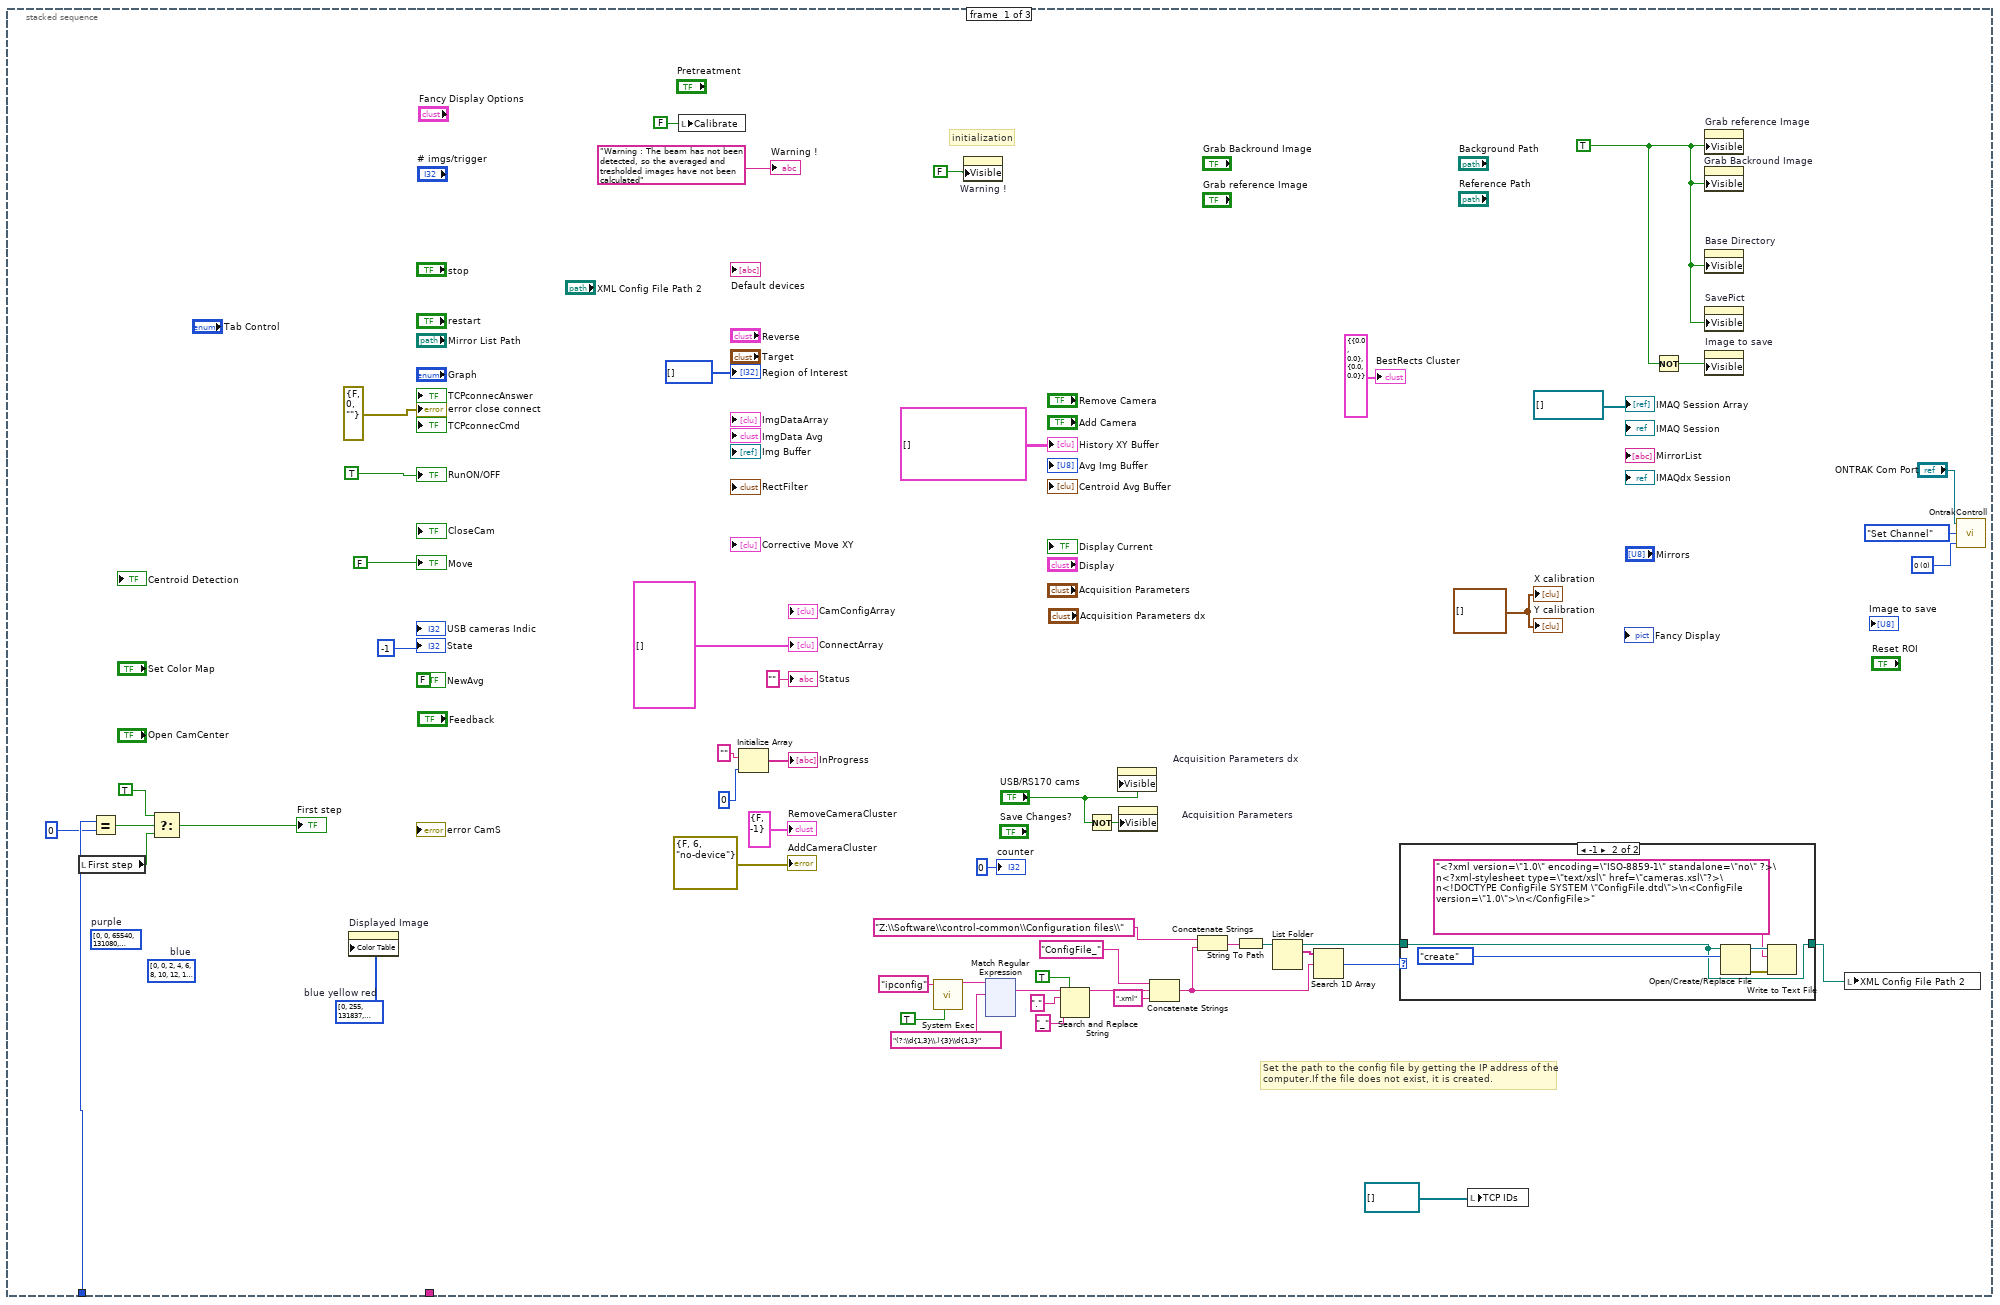
[diagram p8: hidden frame]
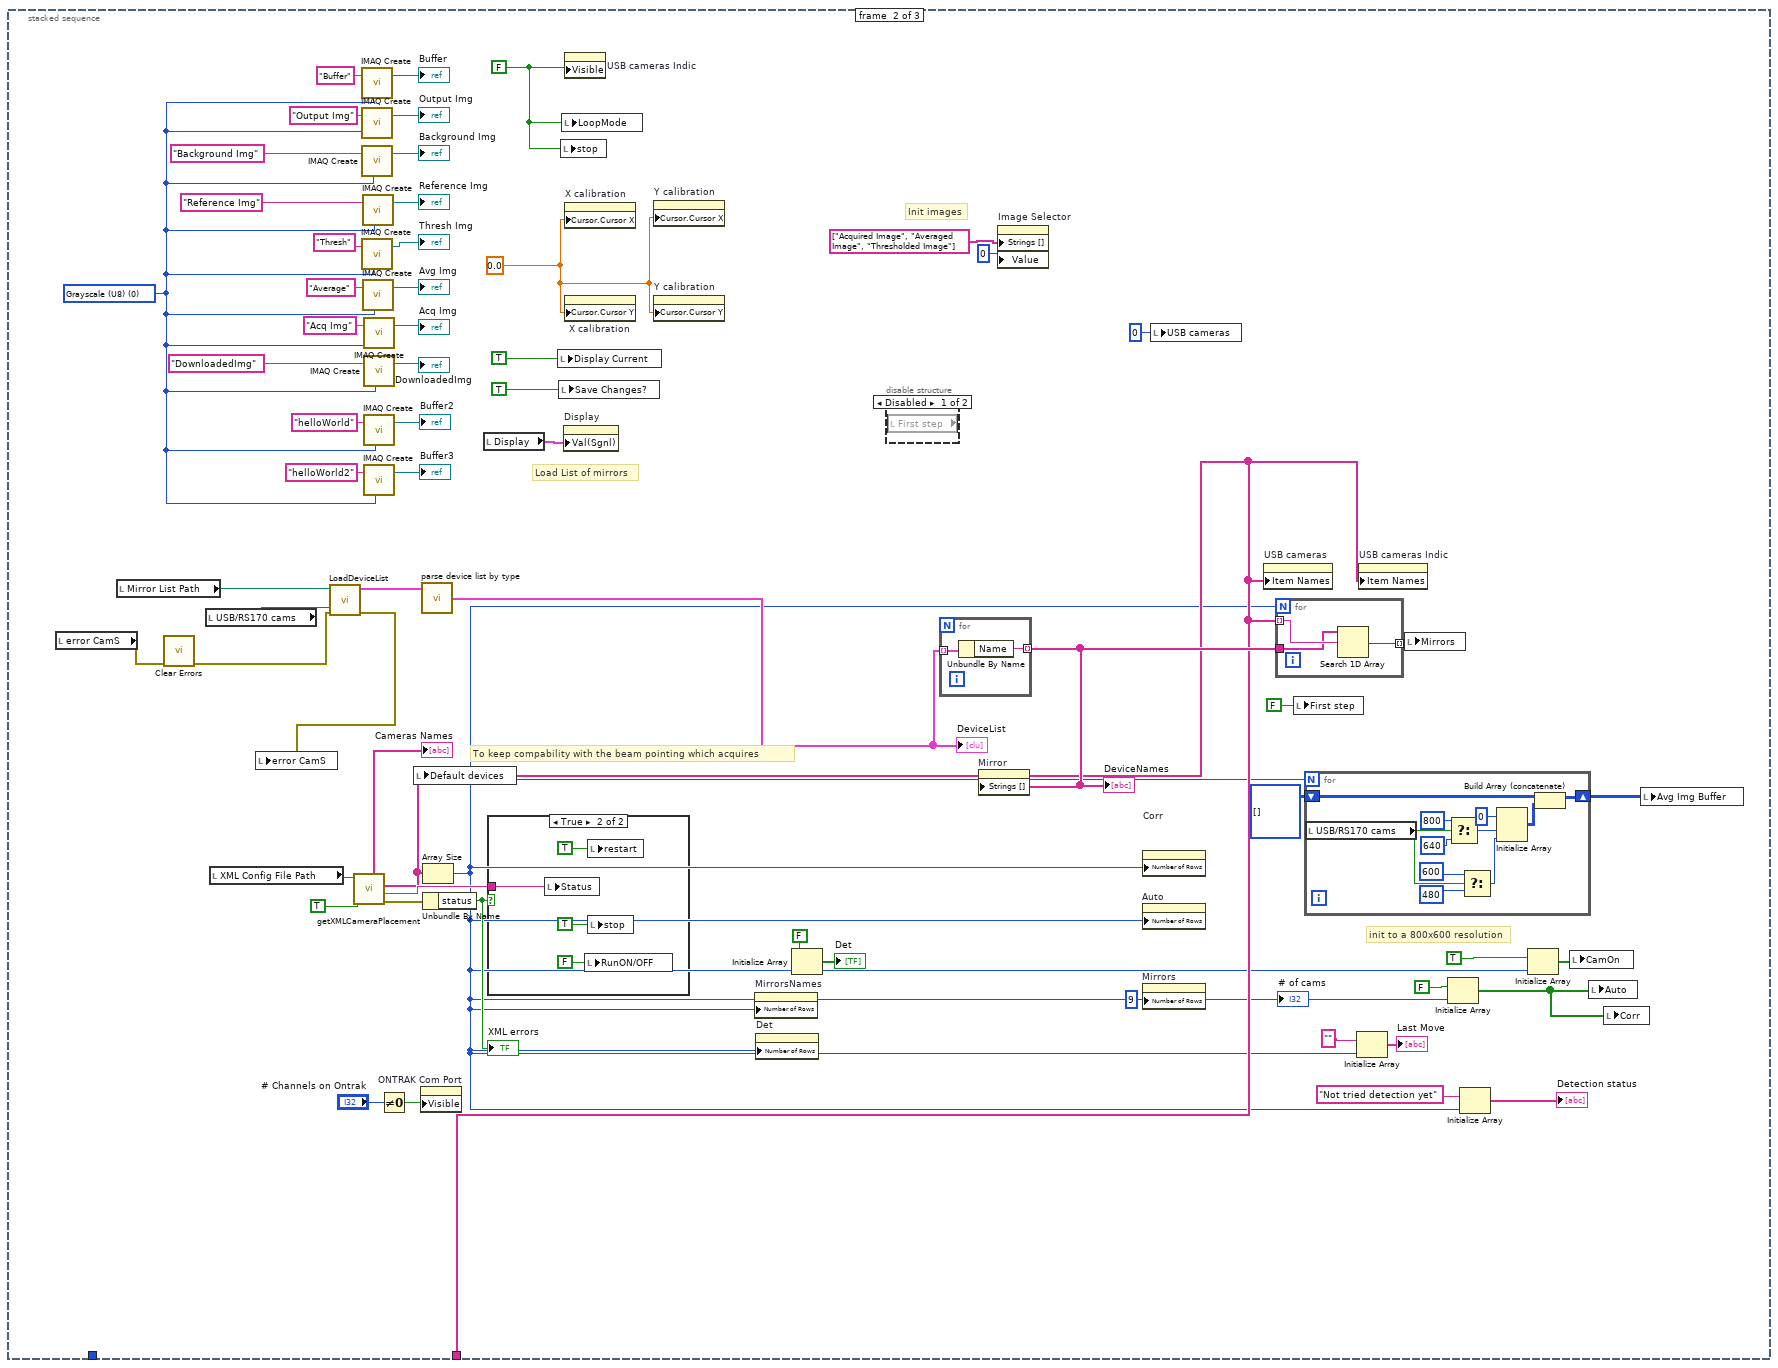
[diagram p10: hidden frame]
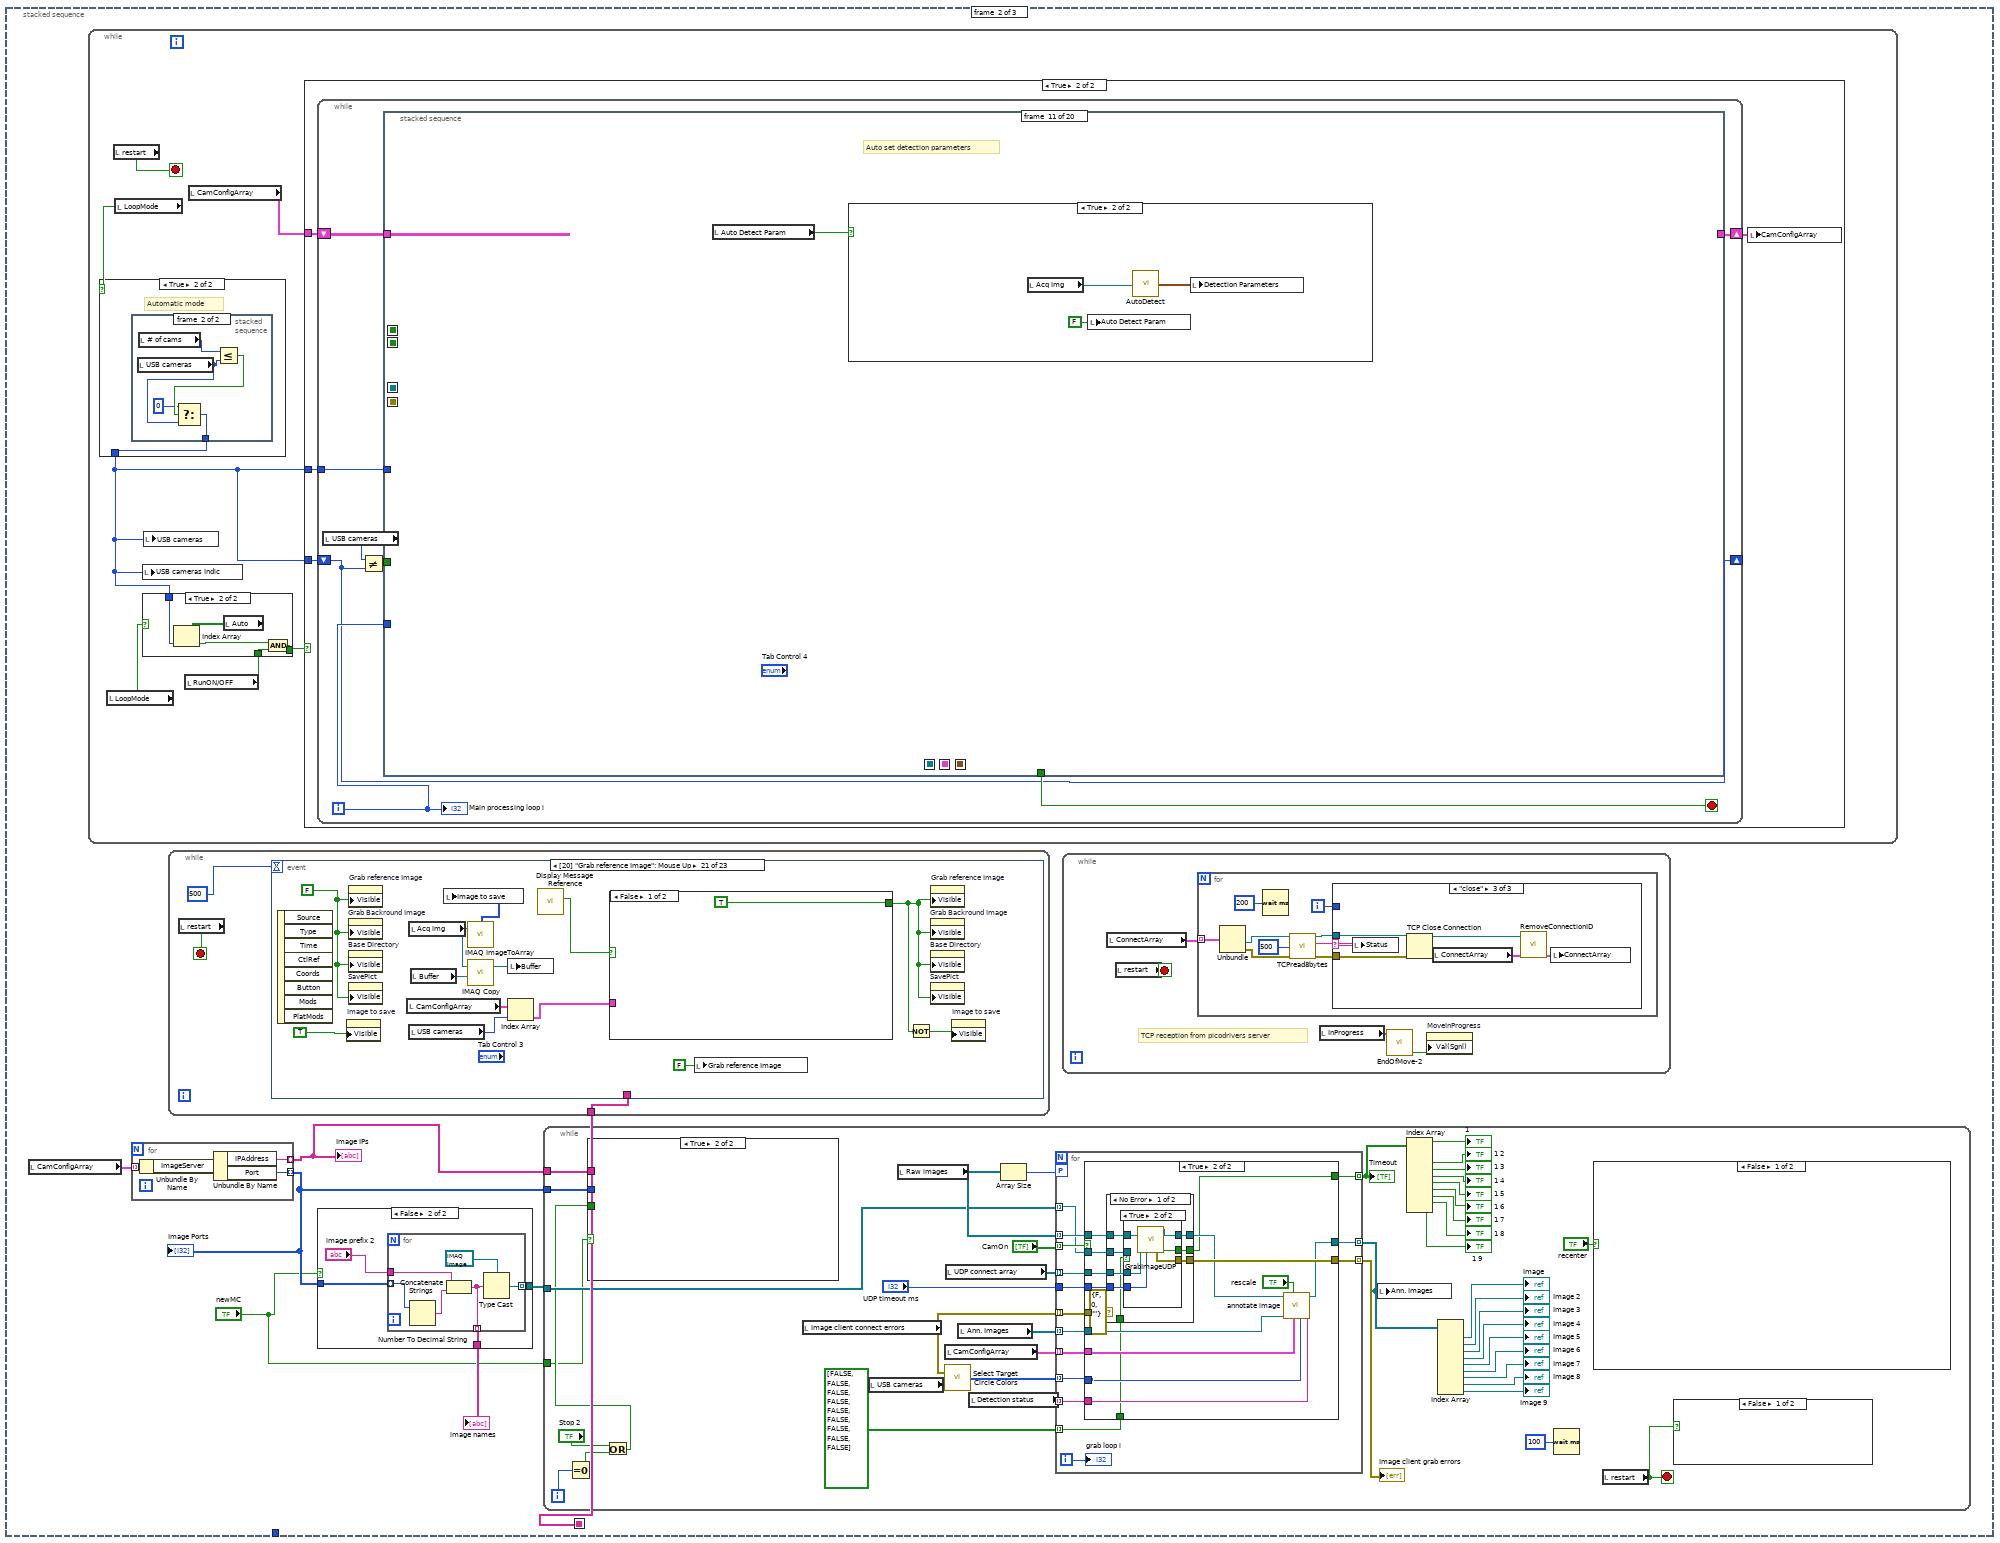
[diagram p13: hidden frame]
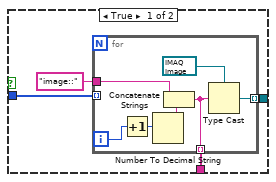
[diagram p14: hidden frame]
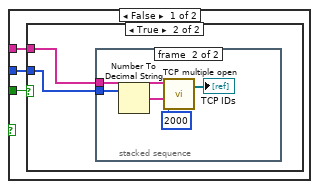
[diagram p15: hidden frame]
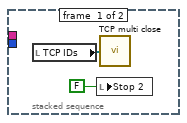
[diagram p17: hidden frame]
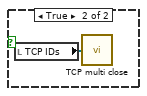
[diagram p18: hidden frame]
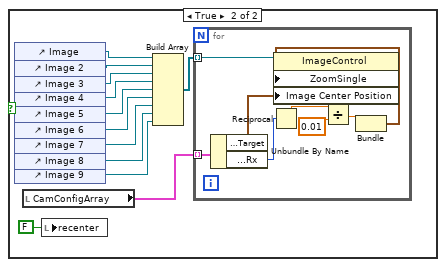
[diagram p19: hidden frame]
diagram:
  (unwired) u32[] [0, 0, 131584, 263168, 394752, 592128, 723712, 855296, 986880, 1118464, 1250048, 1381632, 1579008, 1710592, 1842176, 1973760, 2105345, 2236929, 2368513, 2565889, 2697473, 2829057, 2960641, 3092225, 3223809, 3355393, 3552769, 3684353, 3815937, 3947521, 4079105, 4210689, 4342273, 4539649, 4671233, 4802817, 4934401, 5065985, 5197569, 5329153, 5526529, 5658113, 5789697, 5921281, 6052865, 6184450, 6316034, 6513410, 6644994, 6776578, 6908162, 7039746, 7171330, 7302914, 7500290, 7631874, 7763458, 7895042, 8026626, 8158210, 8289794, 8487170, 8618754, 8750338, 8881922, 9013506, 9145090, 9276674, 9474050, 9605634, 9737218, 9868802, 10000386, 10131970, 10263555, 10460931, 10592515, 10724099, 10855683, 10987267, 11118851, 11250435, 11447811, 11579395, 11710979, 11842563, 11974147, 12105731, 12237315, 12434691, 12566275, 12697859, 12829443, 12961027, 13092611, 13224195, 13421571, 13553155, 13684739, 13816323, 13947907, 14079491, 14211075, 14408452, 14540036, 14671620, 14803204, 14934788, 15066372, 15197956, 15395332, 15526916, 15658500, 15790084, 15921668, 16053252, 16184836, 16382212, 16513796, 16645380, 16776964, 16776452, 16775940, 16775428, 16775172, 16774660, 16774148, 16773636, 16773124, 16772612, 16772356, 16771844, 16771332, 16770820, 16770308, 16769796, 16769540, 16769028, 16768516, 16768004, 16767492, 16766980, 16766468, 16766212, 16765700, 16765188, 16764676, 16764164, 16763652, 16763396, 16762884, 16762372, 16761859, 16761347, 16760835, 16760323, 16760067, 16759555, 16759043, 16758531, 16758019, 16757507, 16757251, 16756739, 16756227, 16755715, 16755203, 16754691, 16754435, 16753923, 16753411, 16752899, 16752387, 16751875, 16751363, 16751107, 16750595, 16750083, 16749571, 16749059, 16748547, 16748291, 16747779, 16747267, 16746755, 16746243, 16745731, 16745475, 16744963, 16744451, 16743939, 16743427, 16742915, 16742403, 16742147, 16741635, 16741123, 16740611, 16740099, 16739587, 16739331, 16738819, 16738307, 16737795, 16737283, 16736771, 16736259, 16736003, 16735491, 16734979, 16734467, 16733955, 16733443, 16733187, 16732675, 16732163, 16731651, 16731139, 16730627, 16730371, 16729858, 16729346, 16728834, 16728322, 16727810, 16727298, 16727042, 16726530, 16726018, 16725506, 16724994, 16724482, 16724226, 16723714, 16723202, 16722690, 16722178, 16721666, 16721154, 16720898, 16720386, 16719874, 16719362, 16718850, 16718338, 16718082, 16717570, 16717058, 16716546, 16716034, 16715522, 16715266, 16714754, 16714242, 16713730, 16448250]
  (unwired) i16[][] array768x1600[1228800 elements] ("Raw image")
  (unwired) i16[][] array768x1600[1228800 elements] ("Raw image")
  (unwired) u32[] [0, 0, 131072, 262144, 393216, 589824, 720896, 851968, 983040, 1114112, 1245184, 1376256, 1572864, 1703936, 1835008, 1966080, 2097152, 2228224, 2359296, 2555904, 2686976, 2818048, 2949120, 3080192, 3211264, 3342336, 3538944, 3670016, 3801088, 3932160, 4063232, 4194304, 4325376, 4521984, 4653056, 4784128, 4915200, 5046272, 5177344, 5308416, 5505024, 5636096, 5767168, 5898240, 6029312, 6160384, 6291456, 6488064, 6619136, 6750208, 6881280, 7012352, 7143424, 7274496, 7471104, 7602176, 7733248, 7864320, 7995392, 8126464, 8257536, 8454144, 8585216, 8716288, 8847360, 8978432, 9109504, 9240576, 9437184, 9568256, 9699328, 9830400, 9961472, 10092544, 10223616, 10420224, 10551296, 10682368, 10813440, 10944512, 11075584, 11206656, 11403264, 11534336, 11665408, 11796480, 11927552, 12058624, 12189696, 12386304, 12517376, 12648448, 12779520, 12910592, 13041664, 13172736, 13369344, 13500416, 13631488, 13762560, 13893632, 14024704, 14155776, 14352384, 14483456, 14614528, 14745600, 14876672, 15007744, 15138816, 15335424, 15466496, 15597568, 15728640, 15859712, 15990784, 16121856, 16318464, 16449536, 16580608, 16711680, 16712192, 16712704, 16713216, 16713728, 16714240, 16714496, 16715008, 16715520, 16716032, 16716544, 16717056, 16717568, 16718080, 16718592, 16719104, 16719360, 16719872, 16720384, 16720896, 16721408, 16721920, 16722432, 16722944, 16723456, 16723968, 16724224, 16724736, 16725248, 16725760, 16726272, 16726784, 16727296, 16727808, 16728320, 16728832, 16729344, 16729600, 16730112, 16730624, 16731136, 16731648, 16732160, 16732672, 16733184, 16733696, 16734208, 16734464, 16734976, 16735488, 16736000, 16736512, 16737024, 16737536, 16738048, 16738560, 16739072, 16739328, 16739840, 16740352, 16740864, 16741376, 16741888, 16742400, 16742912, 16743424, 16743936, 16744448, 16744704, 16745216, 16745728, 16746240, 16746752, 16747264, 16747776, 16748288, 16748800, 16749312, 16749568, 16750080, 16750592, 16751104, 16751616, 16752128, 16752640, 16753152, 16753664, 16754176, 16754432, 16754944, 16755456, 16755968, 16756480, 16756992, 16757504, 16758016, 16758528, 16759040, 16759296, 16759808, 16760320, 16760832, 16761344, 16761856, 16762368, 16762880, 16763392, 16763904, 16764416, 16764672, 16765184, 16765696, 16766208, 16766720, 16767232, 16767744, 16768256, 16768768, 16769280, 16769536, 16770048, 16770560, 16771072, 16771584, 16772096, 16772608, 16773120, 16773632, 16774144, 16774400, 16774912, 16775424, 16775936, 16776448, 16776960, 16448250]
  # "1) Connect on the main port and receive the new port to switch to and connect to that port."
  n1 = flat-sequence {
    frame #0 {
      n2 = call <vilib>:"System Exec.vi"("run minimized? (F)"=TRUE, "command line"="ipconfig") -> ("standard output"=w23:string)  [unwired: 6 in, 3 out]
      n3 = xnode "Match Regular Expression"("input string"=w23, "regular expression"="(?:\\d{1,3}\\.){3}\\d{1,3}") -> ("whole match"=w21:string)  [unwired: 4 in, 4 out]
      n4 = Search and Replace String(replace all?=TRUE ("replace all? (F)"), input string=w21, search string=".", replace string="_" ("replace string (\"\")")) -> (result string=w17:string)  [unwired: 4 in, 3 out]
      n5 = property on="Manual Move" class="Clust"("Visible"=TRUE) -> ()  [unwired: 2 in, 2 out]
      n6 = Concatenate Strings("Z:\\Software\\control-common\\Configuration files\\ConfigFile_" ("replace string (\"\")"), w17, ".xml" ("string")) -> (w15:string)
      n7 = String To Path(string=w15) -> (path=→"XML Config File Path":path)
    }
    frame #1 {
      n8 = while {
        i -> [w137]
        stop <- w138 stop-if-true
        n9 = stacked-sequence {
          seq-local: [w140 _ _] -> [_ w429 _]
          tunnel: [_ _ w1825] -> w138
          tunnel: w137 -> [w139 _ _]
          frame #0 {
            n10 = stacked-sequence {
              tunnel: [_ w330 _] -> w140
              tunnel: w139 -> [w179 _ _]
              frame #0 {
                w142 = u32[] [0, 255, 131837, 263419, 395001, 526583, 658165, 789747, 921329, 1052911, 1184493, 1316075, 1447657, 1579239, 1710820, 1842402, 1973984, 2105566, 2237148, 2368730, 2500312, 2631894, 2828756, 2960338, 3091920, 3223502, 3355084, 3486666, 3618248, 3749830, 3881412, 4012994, 4144576, 4276158, 4407740, 4539322, 4670904, 4802486, 4934068, 5065649, 5197231, 5328813, 5460395, 5591977, 5723559, 5855141, 5986723, 6118305, 6249887, 6381469, 6513051, 6644633, 6776215, 6907797, 7039379, 7170961, 7302543, 7434125, 7565707, 7697289, 7828871, 7960453, 8092035, 8223617, 8355198, 8552060, 8683642, 8815224, 8946806, 9078388, 9209970, 9341552, 9473134, 9604716, 9736298, 9867880, 9999462, 10131044, 10262626, 10394208, 10525790, 10657372, 10788954, 10920536, 11052118, 11183700, 11315282, 11446864, 11578445, 11710027, 11841609, 11973191, 12104773, 12236355, 12367937, 12499519, 12631101, 12762683, 12894265, 13025847, 13157429, 13289011, 13420593, 13552175, 13683757, 13815339, 13946921, 14143783, 14275365, 14406947, 14538529, 14670111, 14801693, 14933274, 15064856, 15196438, 15328020, 15459602, 15591184, 15722766, 15854348, 15985930, 16117512, 16249094, 16380676, 16512258, 16643842, 16775426, 16774914, 16774402, 16773890, 16773378, 16772866, 16772354, 16771842, 16771330, 16770818, 16770306, 16769794, 16769282, 16769026, 16768514, 16768002, 16767490, 16766978, 16766466, 16765954, 16765442, 16764930, 16764418, 16763906, 16763394, 16762882, 16762370, 16761858, 16761346, 16760834, 16760322, 16759809, 16759297, 16758785, 16758273, 16757761, 16757249, 16756737, 16756225, 16755969, 16755457, 16754945, 16754433, 16753921, 16753409, 16752897, 16752385, 16751873, 16751361, 16750849, 16750337, 16749825, 16749313, 16748801, 16748289, 16747777, 16747265, 16746753, 16746241, 16745729, 16745217, 16744705, 16744193, 16743681, 16743425, 16742913, 16742401, 16741889, 16741377, 16740865, 16740353, 16739841, 16739329, 16738817, 16738305, 16737793, 16737281, 16736769, 16736257, 16735745, 16735233, 16734721, 16734209, 16733697, 16733185, 16732673, 16732161, 16731649, 16731137, 16730881, 16730369, 16729857, 16729345, 16728833, 16728321, 16727808, 16727296, 16726784, 16726272, 16725760, 16725248, 16724736, 16724224, 16723712, 16723200, 16722688, 16722176, 16721664, 16721152, 16720640, 16720128, 16719616, 16719104, 16718592, 16718080, 16717824, 16717312, 16716800, 16716288, 16715776, 16715264, 16714752, 16714240, 16713728, 16713216, 16712704, 16712192, 16711680, 16711680]  # blue yellow red
                (unwired) u32[] [0, 0, 65540, 131080, 196620, 262160, 327700, 393240, 458780, 524320, 589860, 589864, 655404, 720944, 786484, 852024, 917564, 983104, 1048644, 1114184, 1179724, 1245264, 1310804, 1376344, 1441884, 1507424, 1572964, 1638504, 1704044, 1704048, 1769588, 1835128, 1900668, 1966208, 2031747, 2097287, 2162827, 2228367, 2293907, 2359447, 2424987, 2490527, 2556067, 2621607, 2687147, 2752687, 2818227, 2883767, 2883771, 2949311, 3014851, 3080391, 3145931, 3211471, 3277011, 3342551, 3408091, 3473631, 3539171, 3604711, 3670251, 3735791, 3801331, 3866871, 3932411, 3997951, 3997951, 4063487, 4129023, 4194559, 4260095, 4325631, 4391167, 4456703, 4522239, 4587775, 4653311, 4718847, 4784383, 4849919, 4915455, 4980991, 5046527, 5112063, 5112063, 5177599, 5243135, 5308671, 5374207, 5439743, 5505279, 5570815, 5636351, 5701887, 5767423, 5832959, 5898495, 5964031, 6029567, 6095103, 6160639, 6226175, 6291711, 6291711, 6357247, 6422783, 6488319, 6553855, 6619391, 6684927, 6750463, 6815999, 6881535, 6947071, 7012607, 7078143, 7143679, 7209215, 7274751, 7340287, 7405823, 7405823, 7471359, 7536895, 7602431, 7667967, 7733503, 7799039, 7864575, 7930111, 7995647, 8061183, 8126719, 8192255, 8257791, 8323327, 8388863, 8519935, 8585471, 8651007, 8716543, 8782079, 8847615, 8913151, 8978687, 9044223, 9109759, 9175295, 9240831, 9306367, 9371903, 9502975, 9568511, 9634047, 9699583, 9765119, 9830655, 9896191, 9961727, 10027263, 10092799, 10158335, 10223871, 10289407, 10354943, 10486015, 10551551, 10617087, 10682623, 10748159, 10813695, 10879231, 10944767, 11010303, 11075839, 11141375, 11206911, 11272447, 11337983, 11469055, 11534591, 11600895, 11667455, 11733759, 11800319, 11866623, 11933183, 11999487, 12066047, 12132351, 12198655, 12265215, 12331519, 12463615, 12529919, 12596479, 12662783, 12729343, 12795647, 12861951, 12928511, 12994815, 13061375, 13127679, 13194239, 13260543, 13392639, 13458943, 13525247, 13591807, 13658111, 13724671, 13790975, 13857535, 13923839, 13990399, 14056703, 14123263, 14189567, 14255871, 14387967, 14454271, 14520831, 14587135, 14653695, 14719999, 14786559, 14852863, 14919167, 14985727, 15052031, 15118591, 15184895, 15251455, 15383295, 15449855, 15516159, 15582463, 15649023, 15715327, 15781887, 15848191, 15914751, 15981055, 16047615, 16113919, 16180223, 16246783, 16378623, 16445183, 16511487, 16578047, 16644351, 16710911, 16777215, 16448250]  # purple
                (unwired) u32[] [0, 0, 2, 4, 6, 8, 10, 12, 14, 16, 18, 20, 22, 24, 26, 28, 30, 32, 34, 36, 38, 40, 42, 44, 46, 48, 50, 52, 54, 56, 58, 60, 62, 64, 66, 68, 70, 72, 74, 76, 78, 80, 82, 84, 86, 88, 90, 92, 94, 96, 98, 100, 102, 104, 106, 108, 110, 112, 114, 116, 118, 120, 122, 124, 126, 128, 130, 132, 134, 136, 138, 140, 142, 144, 146, 148, 150, 152, 154, 156, 158, 160, 162, 164, 166, 168, 170, 172, 174, 176, 178, 180, 182, 184, 186, 188, 190, 192, 194, 196, 198, 200, 202, 204, 206, 208, 210, 212, 214, 216, 218, 220, 222, 224, 226, 228, 230, 232, 234, 236, 238, 240, 242, 244, 246, 248, 250, 252, 255, 131839, 263423, 395007, 526591, 658175, 789759, 921343, 1052927, 1184511, 1316095, 1447679, 1579263, 1710847, 1842431, 1974015, 2105599, 2237183, 2368767, 2500351, 2631935, 2763519, 2895103, 3026687, 3158271, 3289855, 3421439, 3553023, 3684607, 3816191, 3947775, 4079359, 4210943, 4342527, 4474111, 4605695, 4737279, 4868863, 5000447, 5132031, 5263615, 5395199, 5526783, 5658367, 5789951, 5921535, 6053119, 6184703, 6316287, 6447871, 6579455, 6711039, 6842623, 6974207, 7105791, 7237375, 7368959, 7500543, 7632127, 7763711, 7895295, 8026879, 8158463, 8290047, 8421631, 8553215, 8684799, 8816383, 8947967, 9079551, 9211135, 9342719, 9474303, 9605887, 9737471, 9869055, 10000639, 10132223, 10263807, 10395391, 10526975, 10658559, 10790143, 10921727, 11053311, 11184895, 11316479, 11448063, 11579647, 11711231, 11842815, 11974399, 12105983, 12237567, 12369151, 12500735, 12632319, 12763903, 12895487, 13027071, 13158655, 13290239, 13421823, 13553407, 13684991, 13816575, 13948159, 14079743, 14211327, 14342911, 14474495, 14606079, 14737663, 14869247, 15000831, 15132415, 15263999, 15395583, 15527167, 15658751, 15790335, 15921919, 16053503, 16185087, 16316671, 16448255, 16579839, 16777215]  # blue
                w163 = cluster{dbl, dbl}[] [] ("XY Graph")
                w168 = TRUE ("Visible")
                w194 = u16 0 items=["0", "1", "2", "3", "4", "5", "6", "7"] ("Channel\nto Set")
                # "Set the path to the config file by getting the IP address of the computer.If the file does not exist, it is created."
                # "initialization"
                n11 = local read "First step"() -> (w175:bool)
                n12 = Equal?(x=w179, y=0) -> (x = y?=w177:bool)
                n13 = Select(t=TRUE, s=w177, f=w175) -> (s? t:f=→"First step":bool)
                n14 = property on="Displayed Image" class="IntGraph (strict)"("Color Table"=w142) -> ()  [unwired: 2 in, 2 out]
                n15 = local write "Calibrate"(FALSE ("Calibrate")) -> ()
                n16 = Initialize Array("", 0 ("dimension size")) -> (→"InProgress":string[])
                n17 = call <vilib>:"System Exec.vi"("run minimized? (F)"=TRUE, "command line"="ipconfig") -> ("standard output"=w159:string)  [unwired: 6 in, 3 out]
                n18 = property on="Warning !" class="Str"("Visible"=FALSE) -> ()  [unwired: 2 in, 2 out]
                n19 = xnode "Match Regular Expression"("input string"=w159, "regular expression"="(?:\\d{1,3}\\.){3}\\d{1,3}") -> ("whole match"=w157:string)  [unwired: 4 in, 4 out]
                n20 = Search and Replace String(replace all?=TRUE ("replace all? (F)"), input string=w157, search string=".", replace string="_" ("replace string (\"\")")) -> (result string=w153:string)  [unwired: 4 in, 3 out]
                n21 = Not(x="USB/RS170 cams") -> (.not. x?=w165:bool)
                n22 = property on="Acquisition Parameters dx" class="Clust (strict)"("Visible"="USB/RS170 cams") -> ()  [unwired: 2 in, 2 out]
                n23 = property on="Acquisition Parameters" class="Clust (strict)"("Visible"=w165) -> ()  [unwired: 2 in, 2 out]
                n24 = Concatenate Strings("ConfigFile_" ("replace string (\"\")"), w153, ".xml" ("string")) -> (w146:string)
                n25 = Concatenate Strings("Z:\\Software\\control-common\\Configuration files\\" ("replace string (\"\")"), w146) -> (w147:string)
                n26 = String To Path(string=w147) -> (path=w150:path)
                n27 = List Folder(path=w150) -> (path out=w144:path, filenames=w149:string[])  [unwired: 3 in, 2 out]
                n28 = Search 1D Array(1D array=w149, element=w146) -> (index of element=w145:i32)  [unwired: 1 in]
                n29 = case shown="-1" w145 {
                  tunnel: w144 -> [w196 w200]
                  tunnel: [w196 w200] -> w143
                  frame 0, Default {
                  }
                  frame -1 {
                    n30 = Open/Create/Replace File(file path (use dialog)=w200, operation (0:open)=T29."create") -> (refnum out=w198:refnum<file>, error out=w199:errorcluster)  [unwired: 4 in, 1 out]
                    n31 = Write to Text File(file (use dialog)=w198, text="<?xml version=\"1.0\" encoding=\"ISO-8859-1\" standalone=\"no\" ?>\n<?xml-stylesheet type=\"text/xsl\" href=\"cameras.xsl\"?>\n<!DOCTYPE ConfigFile SYSTEM \"ConfigFile.dtd\">\n<ConfigFile version=\"1.0\">\n</ConfigFile>", error in=w199) -> ()  [unwired: 1 in, 3 out]
                  }
                }
                n32 = local write "TCP IDs"(refnum<k5>[] [] ("TCP IDs")) -> ()
                n33 = Not(x=w168) -> (.not. x?=w167:bool)
                n34 = property on="Grab reference Image" class="Bool (strict)"("Visible"=w168) -> ()  [unwired: 2 in, 2 out]
                n35 = property on="Grab Backround Image" class="Bool (strict)"("Visible"=w168) -> ()  [unwired: 2 in, 2 out]
                n36 = property on="Base Directory" class="Path"("Visible"=w168) -> ()  [unwired: 2 in, 2 out]
                n37 = property on="SavePict" class="Bool (strict)"("Visible"=w168) -> ()  [unwired: 2 in, 2 out]
                n38 = property on="Image to save" class="IntGraph (strict)"("Visible"=w167) -> ()  [unwired: 2 in, 2 out]
                n39 = local write "XML Config File Path 2"(w143) -> ()
                n40 = call "OntrakControll.vi"("Channel\nto Set"=w194, "Set/Read"=enum16{"Read Channel", "Set Channel"}."Set Channel", "Comport"="ONTRAK Com Port") -> ()  [unwired: 1 out]
                "Status" <- "" ("status")
                "ConnectArray" <- T7 [] ("ConnectArray")
                "RunON/OFF" <- TRUE ("RunON/OFF")
                "State" <- -1 ("State")
                "error close connect" <- errorcluster {"status"=FALSE, "code"=0, "source"=""} ("error close connect")
                "Move" <- FALSE ("Feedback")
                "NewAvg" <- FALSE ("Feedback")
                "Region of Interest" <- i32[] []
                "History XY Buffer" <- T14 [] ("History XY Buffer")
                "IMAQ Session Array" <- refnum<k11>[] [] ("IMAQ Session Array")
                "Warning !" <- "Warning : The beam has not been detected, so the averaged and tresholded images have not been calculated" ("Warning !")
                "counter" <- 0 ("counter")
                "RemoveCameraCluster" <- cluster{"Remove?":bool, "number":i32} {"Remove?"=FALSE, "number"=-1} ("RemoveCamera")
                "AddCameraCluster" <- T8 {"Add?"=FALSE, "Channel"=6, "Device Name"="no-device"} ("AddCameraCluster")
                "BestRects Cluster" <- T12 {"PreviousCenter"={"X"=0.0, "Y"=0.0}, "CurrentCenter"={"X"=0.0, "Y"=0.0}} ("BestRects Cluster")
                "X calibration" <- w163
                "Y calibration" <- w163
              }
              frame #1 {
                w352 = 0.0 ("Cursor.Cursor Position:Cursor X")
                w314 = T35 0 items=["Grayscale (U8)", "Grayscale (I16)", "Grayscale (SGL)", "Complex (CSG)", "RGB (U32)", "HSL (U32)", "RGB (U64)"] ("Image Type")
                w369 = FALSE ("Enable Feedback")
                # "To keep compability with the beam pointing which acquires"
                # "init to a 800x600 resolution"
                # "Load List of mirrors"
                # "Init images"
                n41 = local read "error CamS"() -> (w336:errorcluster)
                n42 = local read "Mirror List Path"() -> (w351:path)
                n43 = call <vilib>:"Clear Errors.vi"("error in (no error)"=w336) -> ("error out"=w335:errorcluster)  [unwired: 6 in]
                n44 = local read "USB/RS170 cams"() -> (w350:bool)
                n45 = local read "XML Config File Path"() -> (w340:path)
                n46 = call "LoadDeviceList.vi"("error in"=w335, "usb/RS170"=w350, "path to XML document"=w351) -> ("error out"=w349:errorcluster, "DeviceList"=w348:T16)  [unwired: 6 in, 1 out]
                n47 = local write "error CamS"(w349) -> ()
                n48 = call "getXMLCameraPlacement.vi"("usb/watec"=TRUE, "path to XML document"=w340) -> ("error out"=w341:errorcluster, "parse errors"=w342:string, "Default devices"=w330:string[], "Default Cameras Names"=→"Cameras Names":string[])  [unwired: 5 in, 1 out]
                n49 = call "IMAQ Create"("Image Name"="Buffer", "Image Type"=w314) -> ("New Image"=→"Buffer":T1)  [unwired: 2 in, 2 out]
                n50 = call "IMAQ Create"("Image Name"="Output Img", "Image Type"=w314) -> ("New Image"=→"Output Img":T1)  [unwired: 2 in, 2 out]
                n51 = call "IMAQ Create"("Image Name"="Background Img", "Image Type"=w314) -> ("New Image"=→"Background Img":T1)  [unwired: 2 in, 2 out]
                n52 = call "IMAQ Create"("Image Name"="Thresh", "Image Type"=w314) -> ("New Image"=→"Thresh Img":T1)  [unwired: 2 in, 2 out]
                n53 = call "IMAQ Create"("Image Name"="Reference Img", "Image Type"=w314) -> ("New Image"=→"Reference Img":T1)  [unwired: 2 in, 2 out]
                n54 = call "IMAQ Create"("Image Name"="Average", "Image Type"=w314) -> ("New Image"=→"Avg Img":T1)  [unwired: 2 in, 2 out]
                n55 = call "IMAQ Create"("Image Name"="Acq Img", "Image Type"=w314) -> ("New Image"=→"Acq Img":T1)  [unwired: 2 in, 2 out]
                n56 = call "IMAQ Create"("Image Name"="DownloadedImg", "Image Type"=w314) -> ("New Image"=→"DownloadedImg":T1)  [unwired: 2 in, 2 out]
                n57 = call "IMAQ Create"("Image Name"="helloWorld", "Image Type"=w314) -> ("New Image"=→"Buffer2":T1)  [unwired: 2 in, 2 out]
                n58 = call "IMAQ Create"("Image Name"="helloWorld2", "Image Type"=w314) -> ("New Image"=→"Buffer3":T1)  [unwired: 2 in, 2 out]
                n59 = Not Equal To 0?(x="# Channels on Ontrak") -> (x != 0?=w363:bool)
                n60 = local write "Default devices"(w330) -> ()
                n61 = property on="ONTRAK Com Port" class="VISAName"("Visible"=w363) -> ()  [unwired: 2 in, 2 out]
                n62 = call "parse device list by type.vi"("DeviceListin"=w348) -> ("DeviceListout"=w347:T16)  [unwired: 1 in]
                "DeviceList" <- w347
                n63 = Array Size(array=w330) -> (size(s)=w318:i32)
                "# of cams" <- w318
                n64 = Unbundle By Name(w341) -> ("status"=w343:bool)
                "XML errors" <- w343
                n65 = local read "Display"() -> (w365:T26)
                n66 = case shown="True" w343 {
                  tunnel: w342 -> [_ w381]
                  frame False {
                  }
                  frame True {
                    n67 = local write "Status"(w381) -> ()
                    n68 = local write "RunON/OFF"(FALSE ("restart")) -> ()
                    n69 = local write "restart"(TRUE ("restart")) -> ()
                    n70 = local write "stop"(TRUE ("restart")) -> ()
                  }
                }
                n71 = local write "Display Current"(TRUE ("Display Current")) -> ()
                n72 = local write "Save Changes?"(TRUE ("Save Changes")) -> ()
                n73 = local write "stop"(w369) -> ()
                n74 = local write "LoopMode"(w369) -> ()
                n75 = property on="Display" class="Clust (strict)"("Val(Sgnl)"=w365) -> ()  [unwired: 2 in, 2 out]
                n76 = property on="USB cameras Indic" class="LstBox (strict)"("Visible"=w369) -> ()  [unwired: 2 in, 2 out]
                n77 = property on="X calibration" class="XYGraph (strict)"("Cursor.Cursor X"=w352) -> ()  [unwired: 2 in, 2 out]
                n78 = property on="X calibration" class="XYGraph (strict)"("Cursor.Cursor Y"=w352) -> ()  [unwired: 2 in, 2 out]
                n79 = property on="Y calibration" class="XYGraph (strict)"("Cursor.Cursor X"=w352) -> ()  [unwired: 2 in, 2 out]
                n80 = property on="Y calibration" class="XYGraph (strict)"("Cursor.Cursor Y"=w352) -> ()  [unwired: 2 in, 2 out]
                n81 = property on="MirrorsNames" class="Arr (strict)"("Number of Rows"=w318) -> ()  [unwired: 2 in, 2 out]
                n82 = property on="Det" class="Arr (strict)"("Number of Rows"=w318) -> ()  [unwired: 2 in, 2 out]
                n83 = Initialize Array(FALSE, w318) -> (→"Det":bool[])
                n84 = disable-structure shown="Disabled" {
                  frame Disabled {
                    n85 = local read "First step"() -> ()  [unwired: 1 out]
                  }
                  frame Enabled {
                  }
                }
                n86 = for {
                  tunnel: w347 -> [w383] mode=indexing
                  tunnel: [w382] -> w346 mode=indexing
                  n87 = Unbundle By Name(w383) -> ("Name"=w382:string)
                }
                "DeviceNames" <- w346
                n88 = property on="Mirror" class="Ring (strict)"("Strings []"=w346) -> ()  [unwired: 2 in, 2 out]
                n89 = property on="Image Selector" class="Ring (strict)"("Strings []"=string[] ["Acquired Image", "Averaged Image", "Thresholded Image"], "Value"=0) -> ()  [unwired: 2 in, 2 out]
                n90 = property on="Corr" class="Arr (strict)"("Number of Rows"=w318) -> ()  [unwired: 2 in, 2 out]
                n91 = property on="Auto" class="Arr (strict)"("Number of Rows"=w318) -> ()  [unwired: 2 in, 2 out]
                n92 = property on="Mirrors" class="Arr (strict)"("Number of Rows"=u32 9) -> ()  [unwired: 2 in, 2 out]
                n93 = local write "USB cameras"(0 ("USB cameras")) -> ()
                n94 = property on="USB cameras" class="LstBox (strict)"("Item Names"=w330) -> ()  [unwired: 2 in, 2 out]
                n95 = for {
                  N: w318 -> [_]
                  tunnel: [w377] -> w339 mode=indexing
                  tunnel: w330 -> [w376] mode=indexing
                  tunnel: w346 -> [w375]
                  n96 = Search 1D Array(1D array=w375, element=w376) -> (index of element=w377:i32)  [unwired: 1 in]
                }
                n97 = local write "First step"(FALSE ("First step")) -> ()
                n98 = for {
                  N: w318 -> [_]
                  shift-right: [w392] -> w345
                  shift-left: u8[][][] [] -> [w391]
                  n99 = local read "USB/RS170 cams"() -> (w384:bool)
                  n100 = Select(t=800 ("dimension size"), s=w384, f=640 ("dimension size")) -> (s? t:f=w388:i32)
                  n101 = Select(t=600 ("dimension size"), s=w384, f=480 ("dimension size")) -> (s? t:f=w385:i32)
                  n102 = Initialize Array(u8 0 ("element"), w388, w385) -> (w393:u8[][])
                  n103 = Build Array (concatenate)(w391, w393) -> (w392:u8[][][])
                }
                n104 = Initialize Array("" ("time string"), w318) -> (→"Last Move":string[])
                n105 = property on="USB cameras Indic" class="LstBox (strict)"("Item Names"=w330) -> ()  [unwired: 2 in, 2 out]
                n106 = local write "Mirrors"(w339) -> ()
                n107 = Initialize Array(FALSE, w318) -> (w325:bool[])
                n108 = Initialize Array("Not tried detection yet" ("time string"), w318) -> (→"Detection status":string[])
                n109 = Initialize Array(TRUE, w318) -> (w323:bool[])
                n110 = local write "CamOn"(w323) -> ()
                n111 = local write "Auto"(w325) -> ()
                n112 = local write "Corr"(w325) -> ()
                n113 = local write "Avg Img Buffer"(w345) -> ()
              }
              frame #2 {
                w403 = T35 0 items=["Grayscale (U8)", "Grayscale (I16)", "Grayscale (SGL)", "Complex (CSG)", "RGB (U32)", "HSL (U32)", "RGB (U64)"] ("Image Type")
                n114 = local read "DeviceList"() -> (w395:T16)
                n115 = local read "Mirrors"() -> (w405:u8[])
                n116 = call "associate mirrors and cameras.vi"("Mirrors"=w405, "DeviceList"=w395) -> ("CamConfigArray"=w404:T9)  [unwired: 1 in]
                n117 = local write "CamConfigArray"(w404) -> ()
                n118 = for {
                  tunnel: w404 -> [w422] mode=indexing
                  tunnel: [w420] -> w398 mode=indexing
                  tunnel: w403 -> [w407]
                  tunnel: [w418] -> w402 mode=indexing
                  tunnel: ["image servers conn" ("status")] -> w399
                  tunnel: [w414] -> w400 mode=indexing
                  tunnel: [w411] -> w397 mode=indexing
                  tunnel: [w406] -> w396 mode=indexing
                  i -> [w419]
                  n119 = Number To Decimal String(number=w419) -> (decimal integer string=w410:string)  [unwired: 1 in]
                  n120 = Unbundle By Name(w422) -> ("ImageServer"=w421:cluster{"IPAddress":string, "Port":i32})
                  n121 = Concatenate Strings("imageserver" ("string"), w410) -> (w415:string)
                  n122 = call "IMAQ Create"("Image Name"=w415, "Image Type"=w407) -> ("New Image"=w418:T1)  [unwired: 2 in, 2 out]
                  n123 = call "connect udp image server.vi"("ImageServer"=w421) -> ("connection ID"=w414:refnum<k16>, "error out"=w420:errorcluster)  [unwired: 2 in]
                  n124 = Concatenate Strings("imageserver2" ("string"), w410) -> (w412:string)
                  n125 = Concatenate Strings("imageserverAnn" ("string"), w410) -> (w408:string)
                  n126 = call "IMAQ Create"("Image Name"=w412, "Image Type"=w407) -> ("New Image"=w411:T1)  [unwired: 2 in, 2 out]
                  n127 = call "IMAQ Create"("Image Name"=w408, "Image Type"=w407) -> ("New Image"=w406:T1)  [unwired: 2 in, 2 out]
                }
                "Image client connect errors" <- w398
                "Raw images" <- w402
                "UDP connect array" <- w400
                "Images for analysis" <- w397
                "Ann. Images" <- w396
                n128 = local write "Status"("connecting to image servers" ("status")) -> ()
                n129 = local write "Status"(w399) -> ()
              }
            }
          }
          frame #1 {
            n130 = local read "CamConfigArray"() -> (w427:T9)
            n131 = while {
              stop <- w816 stop-if-true
              n132 = local read "LoopMode"() -> (w810:bool)
              n133 = local read "restart"() -> (w816:bool)
              n134 = local read "LoopMode"() -> (w815:bool)
              n135 = case shown="True" w815 {
                tunnel: ["USB cameras" w824] -> w811
                frame False {
                  # "Manual mode"
                }
                frame True {
                  # "Automatic mode"
                  n136 = stacked-sequence {
                    tunnel: [_ w830] -> w824
                    frame #0 {
                      n137 = local read "USB cameras"() -> (w826:i32)
                      n138 = Increment(x=w826) -> (x+1=w825:i32)
                      n139 = local write "USB cameras"(w825) -> ()
                    }
                    frame #1 {
                      n140 = local read "USB cameras"() -> (w828:i32)
                      n141 = local read "# of cams"() -> (w829:i32)
                      n142 = Less Or Equal?(x=w829, y=w828) -> (x <= y?=w831:bool)
                      n143 = Select(t=0, s=w831, f=w828) -> (s? t:f=w830:i32)
                    }
                  }
                }
              }
              n144 = local write "USB cameras Indic"(w811) -> ()
              n145 = local write "USB cameras"(w811) -> ()
              n146 = local read "RunON/OFF"() -> (w813:bool)
              n147 = case shown="True" w810 {
                tunnel: w813 -> [w817 w821]
                tunnel: [w817 w820] -> w812
                tunnel: w811 -> [_ w818]
                frame False {
                }
                frame True {
                  n148 = local read "Auto"() -> (w822:bool[])
                  n149 = Index Array(array=w822, index=w818) -> (element=w819:bool)
                  n150 = And(x=w819, y=w821) -> (x .and. y?=w820:bool)
                }
              }
              n151 = local read "CamConfigArray"() -> (w814:T9)
              n152 = case shown="True" w812 {
                tunnel: w811 -> [_ w836]
                tunnel: w814 -> [_ w835]
                tunnel: w811 -> [_ w833]
                frame False {
                  n153 = Wait (ms)(milliseconds to wait=u32 200 ("millisecond timer value")) -> ()  [unwired: 1 out]
                }
                frame True {
                  n154 = while {
                    tunnel: w836 -> [w844]
                    shift-right: [w840] -> w834
                    shift-left: w835 -> [w841]
                    shift-right: [w837] -> _
                    shift-left: w833 -> [w837]
                    i -> [w842]
                    stop <- w843 stop-if-true
                    n155 = local read "USB cameras"() -> (w839:i32)
                    n156 = Not Equal?(x=w839, y=w837) -> (x != y?=w838:bool)
                    n157 = stacked-sequence {
                      seq-local: [_ _ _ _ _ w1115 _ _ _ _ _ _ _ _ _ _ _ _ _ _] -> [_ _ _ _ _ _ w1190 _ _ _ _ _ _ _ _ _ _ _ _ _]
                      seq-local: [_ _ _ _ _ w1114 _ _ _ _ _ _ _ _ _ _ _ _ _ _] -> [_ _ _ _ _ _ w1189 _ _ _ _ _ _ _ _ _ _ w1578 _ _]
                      seq-local: [_ _ _ _ _ w1113 _ _ _ _ _ _ _ _ _ _ _ _ _ _] -> [_ _ _ _ _ _ w1179 _ _ _ _ _ _ _ w1471 _ _ _ _ _]
                      seq-local: [_ _ _ _ _ w1106 _ _ _ _ _ _ _ _ _ _ _ _ _ _] -> [_ _ _ _ _ _ w1185 _ _ _ _ _ _ _ _ _ _ _ _ _]
                      seq-local: [_ _ _ _ w1045 _ _ _ _ _ _ _ _ _ _ _ _ _ _ _] -> [_ _ _ _ _ w1104 _ _ _ _ _ _ _ _ _ _ _ _ _ _]
                      seq-local: [_ _ _ _ w1065 _ _ _ _ _ _ _ _ _ _ _ _ _ _ _] -> [_ _ _ _ _ w1111 _ _ _ _ _ _ _ _ _ _ _ _ _ _]
                      seq-local: [_ _ _ _ w1064 _ _ _ _ _ _ _ _ _ _ _ _ _ _ _] -> [_ _ _ _ _ w1105 _ _ _ _ _ _ _ _ _ _ _ _ _ _]
                      tunnel: w844 -> [w846 w913 _ w1007 w1048 _ w1170 _ w1265 _ _ _ _ w1411 w1470 w1483 _ _ _ w1737]
                      tunnel: [_ _ _ _ _ _ _ _ _ _ _ _ _ _ _ _ _ _ _ w1734] -> w843
                      tunnel: w842 -> [w847 _ _ _ _ _ _ _ _ _ _ _ _ _ _ _ _ _ _ w1726]
                      tunnel: w841 -> [w845 w914 _ w1016 _ _ _ _ _ _ _ _ _ w1415 _ _ _ _ w1657 w1725]
                      tunnel: [_ _ _ _ _ _ _ _ _ _ _ _ _ _ _ _ _ _ _ w1724] -> w840
                      tunnel: w838 -> [_ _ _ _ _ _ _ _ _ _ _ _ _ _ _ _ _ _ _ w1723]
                      frame #0 {
                        n158 = case shown="0" w847 {
                          tunnel: w846 -> [w895 _]
                          tunnel: w845 -> [w893 _]
                          frame 0 {
                            w889 = T35 0 items=["Grayscale (U8)", "Grayscale (I16)", "Grayscale (SGL)", "Complex (CSG)", "RGB (U32)", "HSL (U32)", "RGB (U64)"] ("Image Type")
                            # "create buffer image"
                            n159 = Index Array(array=w893, index=w895) -> (element=w882:T36)
                            n160 = Unbundle By Name(w882) -> ("CorrectConfig Cluster.Detection Parameters"=w881:T21, "CorrectConfig Cluster.Reverse"=w880:cluster{"Reverse X":bool, "Reverse Y":bool}, "CorrectConfig Cluster.Target"=w879:cluster{"X Target":sgl, "Y Target":sgl}, "CorrectConfig Cluster.Region of Interest"=w878:i32[], "CorrectConfig Cluster.Correction Parameters"=w877:cluster{"X":sgl, "Y":sgl, "Movement Type":u16}, "CorrectConfig Cluster.Reference Path"=w871:path, "CorrectConfig Cluster.Background Path"=w870:path, "CorrectConfig Cluster.Acquisition Parameters"=w876:T27, "CorrectConfig Cluster.XCalibration"=w873:cluster{dbl, dbl}[], "CorrectConfig Cluster.YCalibration"=w872:cluster{dbl, dbl}[], "Name"=→"CurrentName":string, "ImageServer"=→"Current ImageServer":cluster{"IPAddress":string, "Port":i32})
                            n161 = case shown="False" FALSE {
                              tunnel: [w900 w901] -> w896
                              frame False {
                                n162 = local read "Auto"() -> (w900:bool[])
                              }
                              frame True {
                                n163 = local read "Corr"() -> (w901:bool[])
                              }
                            }
                            n164 = Index Array(array=w896, index=w895) -> (element=w894:bool)
                            n165 = local write "Feedback"(w894) -> ()
                            n166 = local write "Y calibration"(w872) -> ()
                            n167 = local write "X calibration"(w873) -> ()
                            n168 = local write "Acquisition Parameters dx"(w876) -> ()
                            n169 = local read "error CamS"() -> (w891:errorcluster)
                            n170 = local read "Mirrors"() -> (w865:u8[])
                            n171 = for {
                              tunnel: w865 -> [w904] mode=indexing
                              tunnel: [w902] -> w848 mode=indexing
                              n172 = local read "DeviceNames"() -> (w903:string[])
                              n173 = Index Array(array=w903, index=w904) -> (element=w902:string)
                            }
                            "MirrorsNames" <- w848
                            n174 = call <vilib>:"Clear Errors.vi"("error in (no error)"=w891) -> ("error out"=w892:errorcluster)  [unwired: 6 in]
                            n175 = local write "Background Path"(w870) -> ()
                            n176 = local write "Acquisition Parameters"(w876) -> ()
                            n177 = local write "Detection Parameters"(w881) -> ()
                            n178 = local write "Target"(w879) -> ()
                            n179 = local read "# imgs to avg"() -> (w890:i32)
                            n180 = local write "Reverse"(w880) -> ()
                            n181 = local write "Reference Path"(w871) -> ()
                            n182 = property on="Region of Interest" class="Arr (strict)"("Val(Sgnl)"=w878) -> ()  [unwired: 2 in, 2 out]
                            n183 = property on="Correction Parameters" class="Clust (strict)"("Val(Sgnl)"=w877) -> ()  [unwired: 2 in, 2 out]
                            n184 = call "Create Image Array.vi"("# of imgs"=w890, "Image Array Base Name"="Buffer", "error in (no error)"=w892, "Image Type"=w889) -> ("Img Array"=w887:T1[], "error out"=w886:errorcluster)  [unwired: 1 in, 9 out]
                            n185 = local write "Img Buffer"(w887) -> ()
                            n186 = local read "Background Img"() -> (w868:T1)
                            n187 = local read "USB/RS170 cams"() -> (w867:bool)
                            n188 = local read "Reference Img"() -> (w869:T1)
                            n189 = local write "error CamS"(w886) -> ()
                            n190 = Initialize Array(T30 {"X Intensity"=[], "Y Intensity"=[], "Max Intensity"=0, "Center"={"X"=0, "Y"=0}, "Radius"={"Rx"=0, "Ry"=0}} ("ImgData"), 0 ("dimension size")) -> (w899:T37)
                            n191 = call "LoadImages.vi"("usb"=w867, "Background Img"=w868, "Background Path"=w870, "Reference Img"=w869, "Reference Path"=w871) -> ()  [unwired: 7 in]
                            n192 = local write "ImgDataArray"(w899) -> ()
                            n193 = Initialize Array("no cam", 9 ("dimension size")) -> (w861:string[])
                            n194 = local read "Switch in"() -> (w885:u32)
                            n195 = Replace Array Subset(array=w861, new element=w848, index=0) -> (w859:string[])
                            n196 = Tick Count (ms)() -> (millisecond timer value=w883:u32)
                            "OpenTime" <- w883
                            n197 = Index Array(array=w859) -> (element #1=w858:string, element #2=w857:string, element #3=w856:string, element #4=w855:string, element #5=w854:string, element #6=w853:string, element #7=w850:string, element #8=w852:string, element #9=w851:string)  [unwired: 9 in]
                            n198 = Subtract(x=w883, y=w885) -> (x-y=→"Switch Time":u32)
                            n199 = local write "Onward"(TRUE ("Onward")) -> ()
                            n200 = property on="Image" class="ImageControl"("Caption.Text"=w858) -> ()  [unwired: 2 in, 2 out]
                            n201 = property on="Image 2" class="ImageControl"("Caption.Text"=w857) -> ()  [unwired: 2 in, 2 out]
                            n202 = property on="Image 3" class="ImageControl"("Caption.Text"=w856) -> ()  [unwired: 2 in, 2 out]
                            n203 = property on="Image 4" class="ImageControl"("Caption.Text"=w855) -> ()  [unwired: 2 in, 2 out]
                            n204 = property on="Image 5" class="ImageControl"("Caption.Text"=w854) -> ()  [unwired: 2 in, 2 out]
                            n205 = property on="Image 6" class="ImageControl"("Caption.Text"=w853) -> ()  [unwired: 2 in, 2 out]
                            n206 = property on="Image 7" class="ImageControl"("Caption.Text"=w850) -> ()  [unwired: 2 in, 2 out]
                            n207 = property on="Image 8" class="ImageControl"("Caption.Text"=w852) -> ()  [unwired: 2 in, 2 out]
                            n208 = property on="Image 9" class="ImageControl"("Caption.Text"=w851) -> ()  [unwired: 2 in, 2 out]
                            "Iteration" <- u32 0 ("Iteration")
                          }
                          frame 1, Default {
                          }
                        }
                      }
                      frame #1 {
                        n209 = local read "Min time between moves (s)"() -> (w912:u32)
                        n210 = local read "MoveInProgress"() -> (w910:bool)
                        n211 = local read "last move time"() -> (w917:u32)
                        n212 = local read "NewAvg"() -> (w906:bool)
                        n213 = Tick Count (ms)() -> (millisecond timer value=w918:u32)
                        n214 = local read "Beam Detected"() -> (w911:bool)
                        n215 = expression code="x*1000" "[ms/s]"(w912) -> (w915:u32)
                        n216 = Subtract(x=w918, y=w917) -> (x-y=w916:u32)
                        n217 = Not(x=w910) -> (.not. x?=w907:bool)
                        n218 = Greater?(x=w916, y=w915) -> (0:w909:bool)
                        n219 = Compound Arithmetic op=AND(w909, "Calibrate", w907, w906) -> (w905:bool)
                        n220 = case shown="True" w905 {
                          tunnel: w914 -> [_ w921]
                          tunnel: w913 -> [_ w920]
                          tunnel: w911 -> [_ w919]
                          frame False {
                            n221 = call "Send Move Command.vi"() -> ()  [unwired: 4 in, 3 out]
                          }
                          frame True {
                            n222 = case shown="True" w919 {
                              tunnel: w921 -> [_ w952]
                              tunnel: w920 -> [_ w951]
                              frame False {
                                n223 = local write "Calibrate"(FALSE ("Calibrate")) -> ()
                              }
                              frame True {
                                w937 = 0.0 ("y")
                                w946 = T38 {"Down"=FALSE, "Up"=FALSE, "Right"=FALSE, "Left"=FALSE, "APulses X"=0, "APulses Y"=0, "Stop"=FALSE} ("Corrective Move")
                                # "picomotor goes onwards and then backwards. And starts this cycle again while going further. All for the purpose of calibrating the motors"
                                n224 = local read "Correction Parameters"() -> (w950:cluster{"X":sgl, "Y":sgl, "Movement Type":u16})
                                n225 = Tick Count (ms)() -> (millisecond timer value=w949:u32)
                                n226 = Index Array(array=w952, index=w951) -> (element=w934:T36)
                                n227 = local write "last move time"(w949) -> ()
                                n228 = local read "Iteration"() -> (w928:u32)
                                n229 = Unbundle By Name(w950) -> ("X"=w948:sgl, "Y"=w947:sgl)
                                n230 = Increment(x=w928) -> (x+1=w923:u32)
                                n231 = Multiply(x=w947, y=w923) -> (x*y=w936:sgl)
                                n232 = Not(x="Onward") -> (.not. x?=w930:bool)
                                n233 = Greater?(x=w923, y=u32 0) -> (0:w932:bool)
                                n234 = Multiply(x=w948, y=w923) -> (x*y=w935:sgl)
                                n235 = Not(x="Onward") -> (.not. x?=w944:bool)
                                n236 = case shown="False" w930 {
                                tunnel: w923 -> [_ w993]
                                frame False {
                                }
                                frame True {
                                n237 = local write "Iteration"(w993) -> ()
                                }
                                }
                                n238 = Bundle By Name(cluster=w946, "Right"="Onward", "Left"=w944, "APulses X"=w935) -> (w943:T38)
                                n239 = local write "Onward"(w930) -> ()
                                n240 = Or(x=w932, y=w930) -> (x .or. y?=w931:bool)
                                n241 = Bundle By Name(cluster=w946, "Up"="Onward", "Down"=w944, "APulses Y"=w936) -> (w942:T38)
                                n242 = local read "ConnectArray"() -> (w954:T7)
                                n243 = local read "Correction Parameters"() -> (w929:cluster{"X":sgl, "Y":sgl, "Movement Type":u16})
                                n244 = Build Array(w943, w942) -> (w941:T39)
                                n245 = Not Equal?(x=w936, y=w937) -> (x != y?=w940:bool)
                                n246 = Not Equal?(x=w935, y=w937) -> (x != y?=w939:bool)
                                n247 = Or(x=w940, y=w939) -> (x .or. y?=w938:bool)
                                n248 = Unbundle By Name(w929) -> ("X"=w927:sgl, "Y"=w926:sgl)
                                n249 = case shown="True" w938 {
                                tunnel: w954 -> [_ w992]
                                tunnel: "webcam" ("client name") -> [_ w989]
                                tunnel: w934 -> [_ w988]
                                tunnel: w941 -> [_ w986]
                                frame False {
                                }
                                frame True {
                                # "Change the direction of the move"
                                n250 = call "Send Move Command.vi"("ConnectArray IN"=w992, "client name"=w989, "CamConfig"=w988, "Move XY"=w986) -> ("ConnectArray Out"=w987:T7, "TCPconnecCmd"=w990:bool, "status"=w991:string)
                                n251 = local write "Status"(w991) -> ()
                                n252 = local write "TCPconnecCmd"(w990) -> ()
                                n253 = local write "ConnectArray"(w987) -> ()
                                }
                                }
                                n254 = Multiply(x=w926, y=w923) -> (x*y=w924:sgl)
                                n255 = Multiply(x=w923, y=w927) -> (x*y=w925:sgl)
                                n256 = case shown="True" w931 {
                                tunnel: w930 -> [_ w960]
                                tunnel: w924 -> [_ w959]
                                tunnel: w925 -> [_ w958]
                                frame False {
                                }
                                frame True {
                                n257 = local read "BestRects Cluster"() -> (w964:T12)
                                n258 = Unbundle By Name(w964) -> ("PreviousCenter"=w962:cluster{"X":dbl, "Y":dbl}, "CurrentCenter"=w961:cluster{"X":dbl, "Y":dbl})
                                n259 = Bundle By Name(cluster=w964, "PreviousCenter"=w961) -> (w963:T12)
                                n260 = Subtract(x=w962, y=w961) -> (x-y=w955:cluster{"X":dbl, "Y":dbl})
                                n261 = local write "BestRects Cluster"(w963) -> ()
                                n262 = Unbundle By Name(w955) -> ("X"=w957:dbl, "Y"=w956:dbl)
                                n263 = case shown="True" w960 {
                                tunnel: w958 -> [w968 w984]
                                tunnel: w959 -> [w967 _]
                                tunnel: w957 -> [w966 w976]
                                tunnel: w956 -> [w965 w975]
                                frame False {
                                n264 = local read "X calibration"() -> (w972:cluster{dbl, dbl}[])
                                n265 = local read "Y calibration"() -> (w969:cluster{dbl, dbl}[])
                                n266 = Bundle(w968, "X"=w966) -> (w971:cluster{sgl, "X":dbl})  [unwired: 1 in]
                                n267 = Bundle(w967, "Y"=w965) -> (w970:cluster{sgl, "Y":dbl})  [unwired: 1 in]
                                n268 = Build Array (concatenate)(w972, w971) -> (w974:cluster{dbl, "X":dbl}[])
                                n269 = Build Array (concatenate)(w969, w970) -> (w973:cluster{dbl, "Y":dbl}[])
                                n270 = local write "X calibration"(w974) -> ()
                                n271 = local write "Y calibration"(w973) -> ()
                                }
                                frame True {
                                n272 = Negate(x=w984) -> (-x=w983:sgl)
                                n273 = Negate(x=w984) -> (-x=w985:sgl)
                                n274 = local read "X calibration"() -> (w981:cluster{dbl, dbl}[])
                                n275 = local read "Y calibration"() -> (w978:cluster{dbl, dbl}[])
                                n276 = Bundle(w983, "X"=w976) -> (w982:cluster{sgl, "X":dbl})  [unwired: 1 in]
                                n277 = Bundle(w985, "Y"=w975) -> (w977:cluster{sgl, "Y":dbl})  [unwired: 1 in]
                                n278 = Build Array (concatenate)(w982, w981) -> (w980:cluster{dbl, "X":dbl}[])
                                n279 = Build Array (concatenate)(w977, w978) -> (w979:cluster{dbl, "Y":dbl}[])
                                n280 = local write "X calibration"(w980) -> ()
                                n281 = local write "Y calibration"(w979) -> ()
                                }
                                }
                                }
                                }
                              }
                            }
                          }
                        }
                      }
                      frame #2 {
                        w999 = FALSE ("Move X?")
                        n282 = local write "Move X"(w999) -> ()
                        n283 = local write "Move Y"(w999) -> ()
                        n284 = case shown="True" "Set Target (Cursor)" {
                          frame False {
                          }
                          frame True {
                            n285 = property on="Displayed Image" class="IntGraph (strict)"("Active Cursor"=u32 0) -> ("Cursor.Cursor Position"=w1006:T40)  [unwired: 2 in, 2 out]
                            n286 = local write "Target"(w1006) -> ()
                          }
                        }
                        n287 = local write "NewAvg"(FALSE ("NewAvg")) -> ()
                        n288 = Tick Count (ms)() -> (millisecond timer value=→"start":u32)
                        n289 = local write "State"(0) -> ()
                        n290 = Initialize Array(T3 {"Down"=FALSE, "Up"=FALSE, "Right"=FALSE, "Left"=FALSE, "APulses X"=0, "APulses Y"=0, "StopButton"=FALSE} ("Corrective Move"), 2 ("dimension size")) -> (w994:T5)
                        n291 = case shown="False" "Set Centroid as Target" {
                          frame False {
                          }
                          frame True {
                            n292 = local read "ImgData Avg"() -> (w1004:T23)
                            n293 = Unbundle By Name(w1004) -> ("Centroid Avg"=w1003:cluster{"X":sgl, "Y":sgl})
                            n294 = local write "Target"(w1003) -> ()
                          }
                        }
                        n295 = local write "Corrective Move XY"(w994) -> ()
                      }
                      frame #3 {
                        # "Send Manual Command"
                        n296 = Index Array(array=w1016, index=w1007) -> (element=w1011:T36)
                        n297 = Bundle By Name(cluster="Manual Move", "APulses X"="Step Size", "APulses Y"="Step Size") -> (w1008:T3)
                        n298 = Unbundle By Name(w1008) -> ("StopButton"=w1017:bool, "Right"=w1021:bool, "Left"=w1020:bool, "Up"=w1019:bool, "Down"=w1018:bool)
                        n299 = local read "Calibrate"() -> (w1013:bool)
                        n300 = Compound Arithmetic op=OR(w1017, w1021, w1020, w1019, w1018) -> (w1015:bool)
                        n301 = Not(x=w1013) -> (.not. x?=w1014:bool)
                        n302 = And(x=w1015, y=w1014) -> (x .and. y?=w1012:bool)
                        n303 = case shown="True" w1012 {
                          tunnel: w1011 -> [_ w1038]
                          tunnel: w1008 -> [_ w1037]
                          tunnel: w1007 -> [_ w1024]
                          frame False {
                          }
                          frame True {
                            n304 = local read "ConnectArray"() -> (w1034:T7)
                            n305 = Initialize Array(w1037, 1 ("dimension size")) -> (w1036:T5)
                            n306 = Get Date/Time In Seconds() -> (seconds since 1Jan1904=w1029:timestamp)
                            n307 = call "Send Move Command.vi"("ConnectArray IN"=w1034, "client name"="webcam", "CamConfig"=w1038, "Move XY"=w1036) -> ("ConnectArray Out"=w1033:T7, "TCPconnecCmd"=w1031:bool, "status"=w1032:string)
                            n308 = local read "Last Move"() -> (w1027:string[])
                            n309 = Get Date/Time String(seconds (now)=w1029, want seconds? (F)=TRUE) -> (time string=w1026:string)  [unwired: 1 in, 1 out]
                            n310 = Replace Array Subset(array=w1027, new element=w1026, index=w1024) -> (w1025:string[])
                            n311 = local write "TCPconnecCmd"(w1031) -> ()
                            n312 = local write "ConnectArray"(w1033) -> ()
                            n313 = local write "Status"(w1032) -> ()
                            n314 = local write "Last Move"(w1025) -> ()
                          }
                        }
                        n315 = local write "State"(1) -> ()
                        n316 = disable-structure shown="Disabled" {
                          frame Disabled {
                            n317 = Bundle By Name("DeviceID"=T31 {"Slot Connector"=0, "IP Adress"="127.0.0.1", "Port"=63410, "Type"="picodriver"}) -> ()  [unwired: 1 in, 1 out]
                          }
                          frame Enabled {
                          }
                        }
                      }
                      frame #4 {
                        # "get image"
                        n318 = local read "Buffer3"() -> (w1043:T1)
                        n319 = local read "USB cameras"() -> (w1040:i32)
                        n320 = local read "Image IPs"() -> (w1041:string[])
                        n321 = while {
                          shift-right: [w1094] -> w1044
                          shift-left: w1043 -> [w1090]
                          tunnel: w1048 -> [w1078]
                          i -> [w1091]
                          stop <- w1093 stop-if-true
                          n322 = local read "USB cameras"() -> (w1089:i32)
                          n323 = local read "DownloadedImg"() -> (w1083:T1)
                          n324 = Equal?(x=w1078, y=w1089) -> (x = y?=w1088:bool)
                          n325 = local read "RunON/OFF"() -> (w1085:bool)
                          n326 = local read "restart"() -> (w1086:bool)
                          n327 = local read "Raw images"() -> (w1079:T1[])
                          n328 = local read "stop"() -> (w1087:bool)
                          n329 = Not(x=w1088) -> (.not. x?=w1081:bool)
                          n330 = local read "Buffer2"() -> (w1080:T1)
                          n331 = call "Update image if new.vi"("Raw images"=w1079, "Image Dst"=w1090, "DownloadedImg"=w1083, "USB cameras"=w1078, "Buffer2"=w1080) -> ("Image Dst Out"=w1094:T1, "Image ok"=w1082:bool)
                          n332 = Not(x=w1085) -> (.not. x?=w1084:bool)
                          n333 = Compound Arithmetic op=OR(w1082, w1087, w1086, w1084, w1081) -> (w1093:bool)
                          n334 = Wait (ms)(milliseconds to wait=u32 100) -> ()  [unwired: 1 out]
                          "#loops waiting for new image" <- w1091
                        }
                        n335 = Index Array(array=w1041, index=w1040) -> (element=→"Image IP":string)
                        n336 = local read "Acq Img"() -> (w1042:T1)
                        n337 = case shown="True" "smooth" {
                          tunnel: w1044 -> [w1072 w1076]
                          tunnel: [w1070 w1075] -> w1047
                          tunnel: w1042 -> [w1071 w1073]
                          frame False {
                            n338 = call "IMAQ Copy"("Image Dst"=w1071, "Image Src"=w1072) -> ("Image Dst Out"=w1070:T1)  [unwired: 4 in, 1 out]
                          }
                          frame True {
                            n339 = call "IMAQ LowPass"("Image Src"=w1076, "Size & Tolerance"="Size & Tolerance", "Image Dst"=w1073) -> ("Image Dst Out"=w1075:T1, "error out"=→"error out":errorcluster)  [unwired: 4 in]
                          }
                        }
                        n340 = local read "Region of Interest"() -> (w1049:i32[])
                        n341 = property class="IMAQImage"(reference=w1047) -> (reference out=w1063:T1, error out=w1062:errorcluster, "ImageSize"=w1061:cluster{"x":i32, "y":i32})  [unwired: 1 in]
                        n342 = Equal?(x=i32[] [0, 0, 0, 0] ("Region of Interest"), y=w1049) -> (x = y?=w1068:bool)
                        n343 = case shown="False" w1068 {
                          tunnel: w1062 -> [w1096 w1100]
                          tunnel: [w1097 w1100] -> w1066
                          tunnel: w1063 -> [w1099 w1101]
                          tunnel: [w1098 w1101] -> w1045
                          tunnel: w1049 -> [w1095 _]
                          frame False {
                            # "Apply ROI"
                            n344 = call "IMAQ Extract"("Optional Rectangle"=w1095, "error in (no error)"=w1096, "Image Src"=w1099) -> ("error out"=w1097:errorcluster, "Image Dst Out"=w1098:T1)  [unwired: 7 in]
                          }
                          frame True {
                          }
                        }
                        n345 = Unbundle By Name(w1061) -> ("x"=w1055:i32, "y"=w1057:i32)
                        n346 = Replace Array Subset(array=i32[] [0, 0, 0, 0] ("Region of Interest"), new element #1=w1055, index #1=2 ("index"), new element #2=w1057, index #2=3 ("index")) -> (→"Img Size":i32[])
                        n347 = local read "Reference Img"() -> (w1053:T1)
                        n348 = local read "Background Img"() -> (w1050:T1)
                        n349 = local read "Output Img"() -> (w1051:T1)
                        n350 = call "Substract Background.vi"("Background"=w1050, "Substract"="Substract", "error in (no error)"=w1066, "Reference"=w1053, "Dest Img"=w1051, "Region of Interest"=w1049, "Image Src"=w1045) -> ("error out"=w1065:errorcluster, "Img Out"=w1052:T1)  [unwired: 2 in]
                        n351 = local write "Output Img"(w1052) -> ()
                        n352 = Unbundle By Name(w1065) -> ("status"=w1067:bool)
                        "IMAQ status" <- w1067
                        n353 = Not(x=w1067) -> (.not. x?=w1064:bool)
                      }
                      frame #5 {
                        # "decide wether or not to do the beam detection"
                        n354 = call "Run Centroid Detection.vi"("Detection Parameters"="Detection Parameters") -> ("Run Detection"=w1109:bool)
                        n355 = Or(x="Auto Detect Param", y=w1109) -> (x .or. y?=w1107:bool)
                        n356 = Not(x="Select ROI") -> (.not. x?=w1108:bool)
                        n357 = local write "Centroid Detection"(w1107) -> ()
                        n358 = And(x=w1107, y=w1108) -> (x .and. y?=w1106:bool)
                        n359 = And(x=w1106, y=w1105) -> (x .and. y?=w1112:bool)
                        n360 = case shown="True" w1112 {
                          tunnel: w1104 -> [w1122 w1134]
                          tunnel: [w1121 w1143] -> w1115
                          tunnel: [_ w1142] -> w1114
                          tunnel: [_ w1137] -> w1113
                          tunnel: w1111 -> [w1120 w1141]
                          tunnel: "Detection Parameters" -> [_ w1124]
                          frame False {
                            w1123 = T35 0 items=["Grayscale (U8)", "Grayscale (I16)", "Grayscale (SGL)", "Complex (CSG)", "RGB (U32)", "HSL (U32)", "RGB (U64)", "Grayscale (U16)"] ("Image Type")
                            n361 = local write "ImgDataArray"(T15 [] ("ImgDataArray")) -> ()
                            n362 = call "IMAQ Cast Image"("Image Type"=w1123, "error in (no error)"=w1120, "Image Src"=w1122) -> ("error out"=w1119:errorcluster, "Image Dst Out"=w1121:T1)  [unwired: 3 in, 4 out]
                            n363 = local write "error CamS"(w1119) -> ()
                            "Beam Detected" <- FALSE ("Beam Detected")
                          }
                          frame True {
                            # "beam detection"
                            n364 = local read "Display"() -> (w1136:T26)
                            n365 = Unbundle By Name(w1136) -> ("Show Best Rect"=w1145:bool, "Show Centroid"=w1144:bool)
                            n366 = local read "Pretreatment"() -> (w1125:bool)
                            n367 = Bundle("Show Best Rect"=w1145, "Show Centroid"=w1144) -> (w1146:T41)  [unwired: 1 out]
                            n368 = call "Beam Detection-v6.vi"("Image Src"=w1134, "Pretreatment"=w1125, "DetectionParameters"=w1124, "error in"=w1141, "Display"=w1146) -> ("Ellipse"=→"Ellipse":T10, "Image Out"=w1135:T1, "Beam is IN"=w1148:bool, "Ellipse edges"=→"Ellipse edges":cluster{"X":sgl, "Y":sgl}[], "Best Rectangle"=w1132:T13, "ImgData"=w1147:T42, "error out"=w1133:errorcluster)  [unwired: 8 in]
                            n369 = case shown="False" w1148 {
                              selector: w1148 -> [_ w1167]
                              tunnel: w1135 -> [w1158 w1166]
                              tunnel: [w1163 w1168] -> w1138
                              tunnel: w1147 -> [_ w1168]
                              tunnel: [w1162 w1167] -> w1126
                              tunnel: [w1153 w1165] -> w1142
                              tunnel: w1133 -> [w1156 w1164]
                              tunnel: [w1161 w1164] -> w1140
                              tunnel: w1146 -> [w1159 _]
                              tunnel: [w1155 w1166] -> w1143
                              tunnel: w1124 -> [w1154 _]
                              tunnel: w1132 -> [_ w1165]
                              tunnel: w1125 -> [w1152 _]
                              frame False {
                                n370 = call "IMAQ GetImageSize"("Image"=w1158) -> ()  [unwired: 1 in, 5 out]
                                n371 = call "IMAQ Clear Overlay"("error in (no error)"=w1156, "Image"=w1158) -> ("error out"=w1157:errorcluster, "Image Out"=w1160:T1)  [unwired: 1 in, 7 out]
                                n372 = call "Beam Detection-v6.vi"("Image Src"=w1160, "Pretreatment"=w1152, "DetectionParameters"=w1154, "error in"=w1157, "Display"=w1159) -> ("Image Out"=w1155:T1, "Beam is IN"=w1162:bool, "Best Rectangle"=w1153:T13, "ImgData"=w1163:T42, "error out"=w1161:errorcluster)  [unwired: 8 in, 2 out]
                              }
                              frame True {
                              }
                            }
                            n373 = local read "Region of Interest"() -> (w1139:i32[])
                            n374 = call-poly "Add ROI Offset.vi"("Region of Interest"=w1139, "ImgData In"=w1138) -> ("ImgData Out"=w1137:T43)  [unwired: 3 in]
                            n375 = case shown="True" w1126 {
                              tunnel: w1140 -> [_ w1151]
                              frame False {
                              }
                              frame True {
                                n376 = local write "error CamS"(w1151) -> ()
                              }
                            }
                            n377 = local read "Beam Detected"() -> (w1129:bool)
                            n378 = Not(x=w1129) -> (.not. x?=w1127:bool)
                            n379 = And(x=w1127, y=w1126) -> (x .and. y?=w1128:bool)
                            n380 = case shown="True" w1128 {
                              selector: w1128 -> [_ w1150]
                              tunnel: w1126 -> [w1149 _]
                              frame False {
                                n381 = local write "Beam Detected"(w1149) -> ()
                              }
                              frame True {
                                n382 = property on="Beam Detected" class="Bool (strict)"("Val(Sgnl)"=w1150) -> ()  [unwired: 2 in, 2 out]
                              }
                            }
                          }
                        }
                        n383 = local write "State"(3 ("State")) -> ()
                      }
                      frame #6 {
                        # "Display current centroid"
                        # "Display current data"
                        n384 = local read "Beam Detected"() -> (w1174:bool)
                        n385 = Select(t="Detected", s=w1174, f=":( Not Detected") -> (s? t:f=w1171:string)
                        n386 = local read "Detection status"() -> (w1176:string[])
                        n387 = local read "Det"() -> (w1178:bool[])
                        n388 = Replace Array Subset(array=w1178, new element=w1174, index=w1170) -> (w1177:bool[])
                        n389 = Replace Array Subset(array=w1176, new element=w1171, index=w1170) -> (w1175:string[])
                        n390 = local read "Auto Detect Param"() -> (w1187:bool)
                        n391 = local write "Det"(w1177) -> ()
                        n392 = local write "Detection status"(w1175) -> ()
                        n393 = Or(x=w1187, y=w1174) -> (x .or. y?=w1188:bool)
                        n394 = And(x=w1185, y=w1188) -> (x .and. y?=w1186:bool)
                        n395 = case shown="True" w1186 {
                          tunnel: w1190 -> [_ w1211]
                          tunnel: w1179 -> [_ w1196]
                          tunnel: w1189 -> [_ w1194]
                          frame False {
                            n396 = local read "Image Selector"() -> (w1192:u16)
                            n397 = Greater?(x=w1192, y=u16 0) -> (0:w1191:bool)
                            n398 = property on="Warning !" class="Str"("Visible"=w1191) -> ()  [unwired: 2 in, 2 out]
                          }
                          frame True {
                            # "Calculate deviation of centroid position from Target"
                            # "add data in buffer"
                            # "add image in buffer"
                            n399 = property on="Warning !" class="Str"("Visible"=FALSE) -> ()  [unwired: 2 in, 2 out]
                            n400 = local write "RectFilter"(w1194) -> ()
                            n401 = Unbundle By Name(w1196) -> ("Center"=w1200:cluster{"X":sgl, "Y":sgl})
                            n402 = local read "ImgDataArray"() -> (w1209:T15)
                            n403 = local read "error CamS"() -> (w1202:errorcluster)
                            n404 = local read "Target"() -> (w1201:cluster{"X Target":sgl, "Y Target":sgl})
                            n405 = local read "Img Buffer"() -> (w1207:T1[])
                            n406 = local read "DeviationArray"() -> (w1199:cluster{"X Centroid":sgl, "Y Centroid":sgl}[])
                            n407 = Subtract(x=w1200, y=w1201) -> (x-y=w1197:cluster{sgl, sgl})
                            "Deviation" <- w1197
                            n408 = Build Array (concatenate)(w1209, w1196) -> (w1206:T15)
                            n409 = Array Size(array=w1207) -> (size(s)=→"ImgBufferSize":i32)
                            n410 = local write "ImgDataArray"(w1206) -> ()
                            n411 = local read "# imgs to avg"() -> (w1205:i32)
                            n412 = Array Size(array=w1206) -> (size(s)=w1203:i32)
                            "# imgs in buffer" <- w1203
                            n413 = call "Copy i_th image to array v2.vi"("Img Array In"=w1207, "Image Src"=w1211, "error in (no error)"=w1202, "Index"=w1203) -> ("error out"=w1210:errorcluster)  [unwired: 10 in, 1 out]
                            n414 = local write "error CamS"(w1210) -> ()
                            n415 = Build Array (concatenate)(w1199, w1197) -> (→"DeviationArray":cluster{"X Centroid":sgl, "Y Centroid":sgl}[])
                            n416 = Equal?(x=w1203, y=w1205) -> (x = y?=w1204:bool)
                            n417 = local write "NewAvg"(w1204) -> ()
                          }
                        }
                        n418 = Unbundle By Name(w1179) -> ("Center"=w1180:cluster{"X":sgl, "Y":sgl}, "Radius"=w1183:cluster{"Rx":sgl, "Ry":sgl}, "Max Intensity"=w1182:sgl)
                        n419 = local read "Img Data"() -> (w1184:T22)
                        n420 = Bundle By Name(cluster=w1184, "Centroid"=w1180, "Radius"=w1183, "Max Intensity"=w1182) -> (→"Img Data":T22)
                        n421 = property on="Displayed Image" class="IntGraph (strict)"("Active Cursor"=u32 3, "Cursor.Cursor Position"=w1180) -> ()  [unwired: 2 in, 2 out]
                      }
                      frame #7 {
                        n422 = local read "ImgDataArray"() -> (w1216:T15)
                        n423 = local read "NewAvg"() -> (w1213:bool)
                        n424 = local read "error CamS"() -> (w1218:errorcluster)
                        n425 = local read "Img Buffer"() -> (w1217:T1[])
                        n426 = Array Size(array=w1216) -> (size(s)=w1215:i32)
                        n427 = local write "State"(5) -> ()
                        n428 = Not Equal To 0?(x=w1215) -> (x != 0?=w1212:bool)
                        n429 = And(x=w1212, y=w1213) -> (x .and. y?=w1214:bool)
                        n430 = case shown="True" w1214 {
                          tunnel: w1218 -> [_ w1243]
                          tunnel: w1217 -> [_ w1242]
                          tunnel: w1216 -> [_ w1241]
                          frame False {
                          }
                          frame True {
                            # "Display Avg Data"
                            # "average image"
                            # "sort images and average data"
                            # "averaging"
                            n431 = local read "USB/RS170 cams"() -> (w1224:bool)
                            n432 = call "RemoveBadSpotImage-v3.vi"("error in"=w1243, "ImgDataArray"=w1241, "Img Array In"=w1242) -> ("error out"=w1239:errorcluster, "Averages"=w1235:T23, "Img Array Sorted"=w1227:T1[])  [unwired: 1 in, 1 out]
                            n433 = local read "Avg Img"() -> (w1240:T1)
                            n434 = property on="Warning !" class="Str"("Visible"=FALSE) -> ()  [unwired: 2 in, 2 out]
                            n435 = call "Greyscale Image Averager3.vi"("Img Array IN"=w1227, "Image Dst In"=w1240, "usb"=w1224, "error in (no error)"=w1239) -> ("Img Array Out"=w1230:T1[], "Image Dst Out"=w1231:T1, "error out"=w1229:errorcluster)  [unwired: 9 in]
                            n436 = call "IMAQ Dispose Buffer.vi"("error in"=w1229, "Img Buffer In"=w1230) -> ("error out"=w1228:errorcluster)  [unwired: 1 in]
                            n437 = case shown="True" "Avg data/ data of avg img" {
                              tunnel: w1228 -> [w1246 w1264]
                              tunnel: w1231 -> [w1244 w1258]
                              tunnel: [w1246 w1257] -> w1236
                              tunnel: [w1245 w1252] -> w1221
                              tunnel: w1235 -> [w1245 _]
                              tunnel: [w1244 w1250] -> w1226
                              frame False {
                              }
                              frame True {
                                n438 = local read "Display"() -> (w1262:T26)
                                n439 = local read "Detection Parameters"() -> (w1263:T21)
                                n440 = Unbundle By Name(w1262) -> ("Show Best Rect"=w1261:bool, "Show Centroid"=w1260:bool)
                                n441 = local read "Pretreatment"() -> (w1247:bool)
                                n442 = Bundle("Show Best Rect"=w1261, "Show Centroid"=w1260) -> (w1259:T41)  [unwired: 1 out]
                                n443 = call "Beam Detection-v6.vi"("Image Src"=w1258, "Pretreatment"=w1247, "DetectionParameters"=w1263, "error in"=w1264, "Display"=w1259) -> ("Ellipse"=w1249:T10, "Image Out"=w1250:T1, "Ellipse edges"=w1248:cluster{"X":sgl, "Y":sgl}[], "ImgData"=w1256:T42, "error out"=w1257:errorcluster)  [unwired: 8 in, 2 out]
                                n444 = local write "Ellipse"(w1249) -> ()
                                n445 = local write "Ellipse edges"(w1248) -> ()
                                n446 = Unbundle By Name(w1256) -> ("Max Intensity"=w1254:u8, "Centroid"=w1251:cluster{"X":i32, "Y":i32}, "Radius"=w1253:cluster{"Rx":i32, "Ry":i32})
                                n447 = local read "ImgData Avg"() -> (w1255:T23)
                                n448 = Bundle By Name(cluster=w1255, "Max Intensity Avg"=w1254, "Centroid Avg"=w1251, "Radius Avg"=w1253) -> (w1252:T23)
                              }
                            }
                            n449 = local read "Detection Parameters"() -> (w1233:T21)
                            n450 = Unbundle By Name(w1233) -> ("Treshold"=w1232:u8)
                            n451 = local read "Thresh Img"() -> (w1238:T1)
                            n452 = call "Threshold Img v2.vi"("error in (no error)"=w1236, "Threshold"=w1232, "Img Dst"=w1238, "Img Src"=w1226) -> ("error out"=w1237:errorcluster)  [unwired: 6 in, 1 out]
                            n453 = local write "error CamS"(w1237) -> ()
                            n454 = local write "ImgData Avg"(w1221) -> ()
                            n455 = Unbundle By Name(w1221) -> ("Centroid Avg"=w1220:cluster{"X":sgl, "Y":sgl})
                            n456 = local read "BestRects Cluster"() -> (w1222:T12)
                            n457 = Bundle By Name(cluster=w1222, "CurrentCenter"=w1220) -> (w1223:T12)
                            n458 = local write "BestRects Cluster"(w1223) -> ()
                          }
                        }
                      }
                      frame #8 {
                        # "image saving"
                        n459 = local read "NewAvg"() -> (w1267:bool)
                        n460 = local read "ImgDataArray"() -> (w1271:T15)
                        n461 = Array Size(array=w1271) -> (size(s)=w1270:i32)
                        n462 = Not Equal To 0?(x=w1270) -> (x != 0?=w1268:bool)
                        n463 = Compound Arithmetic op=AND("SavePict", w1268, w1267) -> (w1266:bool)
                        n464 = case shown="True" w1266 {
                          tunnel: w1265 -> [_ w1272]
                          frame False {
                          }
                          frame True {
                            n465 = stacked-sequence {
                              seq-local: [w1274 _] -> [_ w1300]
                              tunnel: w1272 -> [_ w1287]
                              frame #0 {
                                n466 = local read "MirrorsNames"() -> (w1273:string[])
                                n467 = for {
                                tunnel: [w1276] -> w1274 mode=indexing
                                tunnel: w1273 -> [w1275] mode=indexing
                                n468 = Search and Replace String(input string=w1275, search string=":", replace string="-" ("replace string (\"\")")) -> (result string=w1279:string)  [unwired: 5 in, 3 out]
                                n469 = Build Path(base path="Base Directory", name or relative path=w1279) -> (appended path=w1278:path)
                                n470 = List Folder(path="Base Directory") -> (folder names=w1280:string[])  [unwired: 3 in, 3 out]
                                n471 = Search 1D Array(1D array=w1280, element=w1279) -> (index of element=w1277:i32)  [unwired: 1 in]
                                n472 = case shown="-1" w1277 {
                                tunnel: w1278 -> [w1284 w1286]
                                tunnel: [w1284 w1285] -> w1276
                                frame 0, Default {
                                }
                                frame -1 {
                                n473 = Create Folder(path (use dialog)=w1286) -> (created path=w1285:path)  [unwired: 2 in, 2 out]
                                }
                                }
                                }
                              }
                              frame #1 {
                                n474 = local read "Avg Img"() -> (w1292:T1)
                                n475 = local read "Beam Detected"() -> (w1304:bool)
                                n476 = call "IMAQ Create"("Image Name"="toDeinterlace") -> ("New Image"=w1296:T1)  [unwired: 4 in, 1 out]
                                n477 = Index Array(array=w1300, index=w1287) -> (element=w1299:path)
                                n478 = Select(t="Beam In.png" ("string"), s=w1304, f="Beam Out.png" ("string")) -> (s? t:f=w1302:string)
                                n479 = call "IMAQ Copy"("Image Dst"=w1296, "Image Src"=w1292) -> ("Image Dst Out"=w1288:T1)  [unwired: 4 in, 1 out]
                                n480 = local read "Main processing loop i"() -> (w1308:i32)
                                n481 = Path To String(path=w1299) -> (string=w1298:string)
                                n482 = Number To Decimal String(number=w1308) -> (decimal integer string=w1307:string)  [unwired: 1 out]
                                n483 = call "IMAQ Interlace"("Image Even"=w1288, "Image Odd"=w1288, "Image Frame"=w1288, "Interlace/Separate (Interlace)"=TRUE) -> ("Image Odd Out"=→"Image Odd Out":T1, "Image Even Out"=w1290:T1)  [unwired: 1 in, 2 out]
                                n484 = Concatenate Strings(w1298, "\\" ("string"), w1307, w1302) -> (w1309:string)
                                n485 = Select(t=w1290, s="Boolean", f=w1292) -> (s? t:f=w1291:T1)
                                n486 = String To Path(string=w1309) -> (path=w1306:path)
                                n487 = call "IMAQ Write Image And Vision Info"("File Path"=w1306, "Image"=w1291) -> ("error out"=→"SaveImgError":errorcluster)  [unwired: 2 in, 7 out]
                              }
                            }
                          }
                        }
                      }
                      frame #9 {
                        # "Calclulate average values for correction"
                        n488 = local read "NewAvg"() -> (w1312:bool)
                        n489 = case shown="True" w1312 {
                          tunnel: [w1314 w1324] -> w1311
                          tunnel: [w1314 w1318] -> w1310
                          frame False {
                            w1314 = cluster{bool, bool} {FALSE, FALSE}
                          }
                          frame True {
                            n490 = local read "ImgData Avg"() -> (w1325:T23)
                            n491 = local read "ImgData Avg"() -> (w1327:T23)
                            n492 = local read "Initiate Correction Range"() -> (w1321:i16)
                            n493 = Unbundle By Name(w1325) -> ("Centroid Avg"=w1328:cluster{"X":sgl, "Y":sgl})
                            n494 = Unbundle By Name(w1327) -> ("Radius Avg"=w1326:cluster{"Rx":sgl, "Ry":sgl})
                            n495 = local read "Target"() -> (w1322:cluster{"X Target":sgl, "Y Target":sgl})
                            n496 = local read "DeviationArray"() -> (w1315:cluster{"X Centroid":sgl, "Y Centroid":sgl}[])
                            n497 = Divide(x=w1321, y=sgl 100.0) -> (x/y=w1317:sgl)
                            n498 = Subtract(x=w1328, y=w1322) -> (x-y=w1330:cluster{sgl, sgl})
                            "Avg Deviation" <- w1330
                            n499 = Multiply(x=w1326, y=w1317) -> (x*y=w1323:cluster{"Rx":sgl, "Ry":sgl})
                            n500 = Absolute Value(x=w1330) -> (abs(x)=w1329:cluster{sgl, sgl})
                            n501 = Greater?(x=w1329, y=w1323) -> (0:w1324:cluster{bool, bool})
                            n502 = call "percent true of DeviationArray.vi"("DeviationArray"=w1315, "Threshold"=w1323) -> ("% XY State True"=w1320:cluster{dbl, dbl})  [unwired: 7 out]
                            "% XY State True" <- w1320
                            n503 = Greater?(x=w1320, y="Threshold [%]") -> (0:w1318:cluster{bool, bool})
                          }
                        }
                        "Out of Range?" <- w1311
                        "%Out of Range" <- w1310
                        n504 = local write "State"(7) -> ()
                      }
                      frame #10 {
                        # "Auto set detection parameters"
                        n505 = local read "Auto Detect Param"() -> (w1331:bool)
                        n506 = case shown="True" w1331 {
                          frame False {
                          }
                          frame True {
                            n507 = local read "Acq Img"() -> (w1333:T1)
                            n508 = local write "Auto Detect Param"(FALSE ("Auto Detect Param")) -> ()
                            n509 = call "AutoDetect.vi"("Image"=w1333) -> ("Detection Parameters Out"=w1334:T21)
                            n510 = local write "Detection Parameters"(w1334) -> ()
                          }
                        }
                      }
                      frame #11 {
                        # "Decide wether or not to initiate a correction sequence"
                        n511 = local read "Feedback"() -> (w1335:bool)
                        n512 = local read "NewAvg"() -> (w1336:bool)
                        n513 = And(x=w1335, y=w1336) -> (x .and. y?=w1337:bool)
                        n514 = case shown="True" w1337 {
                          frame False {
                          }
                          frame True {
                            n515 = local read "%Out of Range"() -> (w1339:cluster{"Dev. X":bool, "Dev. Y":bool})
                            n516 = local read "Out of Range?"() -> (w1343:cluster{"Dev. X":bool, "Dev. Y":bool})
                            n517 = And(x="use Avg Out of Range?", y=w1343) -> (x .and. y?=w1342:cluster{"Dev. X":bool, "Dev. Y":bool})
                            n518 = And(x="use % Out of Range", y=w1339) -> (x .and. y?=w1345:cluster{"Dev. X":bool, "Dev. Y":bool})
                            n519 = Compound Arithmetic op=OR(w1342, w1345) -> (w1347:cluster{"Dev. X":bool, "Dev. Y":bool})
                            n520 = Unbundle(w1347) -> ("Dev. X"=→"Move X":bool, "Dev. Y"=→"Move Y":bool)
                          }
                        }
                        n521 = local write "State"(9) -> ()
                      }
                      frame #12 {
                        # "Calculate required move parameters to correct beam pointing"
                        n522 = Unbundle By Name("Correction Parameters") -> ("Movement Type"=w1351:u16, "X"=w1349:sgl, "Y"=w1348:sgl)
                        n523 = local read "Corrective Move XY"() -> (w1354:T5)
                        n524 = local read "Avg Deviation"() -> (w1355:cluster{sgl, sgl})
                        n525 = local read "Move Y"() -> (w1356:bool)
                        n526 = local read "Move X"() -> (w1357:bool)
                        n527 = Unbundle(w1355) -> (w1359:sgl, w1358:sgl)
                        n528 = case shown="True" w1357 {
                          tunnel: w1359 -> [w1391 _]
                          tunnel: w1351 -> [w1390 _]
                          tunnel: w1354 -> [w1386 w1398]
                          tunnel: [w1387 w1398] -> w1353
                          tunnel: w1349 -> [w1381 _]
                          frame True {
                            n529 = case shown="1" w1390 {
                              tunnel: w1391 -> [_ w1395]
                              tunnel: [w1393 w1396] -> w1382
                              tunnel: w1381 -> [w1393 _]
                              frame 0, Default {
                              }
                              frame 1 {
                                n530 = local read "X calibration"() -> (w1397:cluster{dbl, dbl}[])
                                n531 = Negate(x=w1395) -> (-x=w1394:sgl)
                                n532 = call "FindNrSteps.vi"("X calibration"=w1397, "pixels"=w1394) -> ("NrSteps"=w1396:dbl)
                              }
                            }
                            n533 = Index Array(array=w1386, index=0) -> (element=w1388:T3)
                            n534 = Greater Or Equal To 0?(x=w1391) -> (x >= 0?=w1380:bool)
                            n535 = Absolute Value(x=w1382) -> (abs(x)=w1383:dbl)
                            n536 = Not(x=w1380) -> (.not. x?=w1392:bool)
                            n537 = Bundle By Name(cluster=w1388, "Left"=w1380, "Right"=w1392, "APulses X"=w1383) -> (w1385:T3)
                            n538 = Replace Array Subset(array=w1386, new element=w1385, index=0) -> (w1387:T5)
                          }
                          frame False {
                          }
                        }
                        n539 = case shown="True" w1356 {
                          tunnel: w1358 -> [w1373 _]
                          tunnel: w1351 -> [w1372 _]
                          tunnel: w1353 -> [w1368 w1379]
                          tunnel: [w1367 w1379] -> w1352
                          tunnel: w1348 -> [w1363 _]
                          frame True {
                            n540 = case shown="1" w1372 {
                              tunnel: w1373 -> [_ w1376]
                              tunnel: [w1374 w1377] -> w1365
                              tunnel: w1363 -> [w1374 _]
                              frame 0, Default {
                              }
                              frame 1 {
                                n541 = local read "Y calibration"() -> (w1378:cluster{dbl, dbl}[])
                                n542 = Negate(x=w1376) -> (-x=w1375:sgl)
                                n543 = call "FindNrSteps.vi"("X calibration"=w1378, "pixels"=w1375) -> ("NrSteps"=w1377:dbl)
                              }
                            }
                            n544 = Absolute Value(x=w1365) -> (abs(x)=w1364:dbl)
                            n545 = Greater Or Equal To 0?(x=w1373) -> (x >= 0?=w1361:bool)
                            n546 = Not(x=w1361) -> (.not. x?=w1362:bool)
                            n547 = Index Array(array=w1368, index=1) -> (element=w1369:T3)
                            n548 = Bundle By Name(cluster=w1369, "Down"=w1362, "Up"=w1361, "APulses Y"=w1364) -> (w1366:T3)
                            n549 = Replace Array Subset(array=w1368, new element=w1366, index=1) -> (w1367:T5)
                          }
                          frame False {
                          }
                        }
                        n550 = local write "Corrective Move XY"(w1352) -> ()
                        n551 = local write "State"(10) -> ()
                      }
                      frame #13 {
                        # "Send Corrective Move command"
                        n552 = local read "Corrective Move XY"() -> (w1424:T5)
                        n553 = local read "last move time"() -> (w1422:u32)
                        n554 = Index Array(array=w1415, index=w1411) -> (element=w1416:T36)
                        n555 = Tick Count (ms)() -> (millisecond timer value=w1423:u32)
                        n556 = expression code="x*1000" "[ms/s]"("Min time between moves (s)") -> (w1419:u32)
                        n557 = for {
                          tunnel: w1424 -> [w1433] mode=indexing
                          shift-right: [w1427] -> w1399
                          shift-left: FALSE -> [w1428]
                          n558 = Unbundle By Name(w1433) -> ("Right"=w1432:bool, "Left"=w1431:bool, "Up"=w1430:bool, "Down"=w1429:bool, "StopButton"=w1426:bool)
                          n559 = Compound Arithmetic op=OR(w1428, w1432, w1431, w1430, w1429, w1426) -> (w1427:bool)
                        }
                        "conn req" <- w1399
                        n560 = Subtract(x=w1423, y=w1422) -> (x-y=w1421:u32)
                        n561 = Greater?(x=w1421, y=w1419) -> (0:w1418:bool)
                        n562 = local read "Calibrate"() -> (w1414:bool)
                        n563 = Not(x=w1414) -> (.not. x?=w1413:bool)
                        n564 = local read "Last Move"() -> (w1410:string[])
                        n565 = And(x=w1418, y=w1399) -> (x .and. y?=w1412:bool)
                        n566 = And(x=w1413, y=w1412) -> (x .and. y?=w1400:bool)
                        "will move" <- w1400
                        n567 = case shown="True" w1400 {
                          tunnel: w1416 -> [_ w1440]
                          tunnel: w1424 -> [_ w1443]
                          tunnel: w1411 -> [_ w1435]
                          frame False {
                          }
                          frame True {
                            n568 = Get Date/Time In Seconds() -> (seconds since 1Jan1904=w1439:timestamp)
                            n569 = local read "Last Move"() -> (w1437:string[])
                            n570 = Get Date/Time String(seconds (now)=w1439, want seconds? (F)=TRUE) -> (time string=w1436:string)  [unwired: 1 in, 1 out]
                            n571 = local read "ConnectArray"() -> (w1442:T7)
                            n572 = Replace Array Subset(array=w1437, new element=w1436, index=w1435) -> (w1434:string[])
                            n573 = local write "Last Move"(w1434) -> ()
                            n574 = Tick Count (ms)() -> (millisecond timer value=→"last move time":u32)
                            n575 = stacked-sequence {
                              tunnel: w1443 -> [w1451 _ _]
                              tunnel: w1442 -> [w1450 _ _]
                              tunnel: "webcam" ("client name") -> [w1449 _ _]
                              tunnel: w1440 -> [w1448 _ _]
                              frame #0 {
                                n576 = call "Send Move Command.vi"("ConnectArray IN"=w1450, "client name"=w1449, "CamConfig"=w1448, "Move XY"=w1451) -> ("ConnectArray Out"=w1447:T7, "TCPconnecCmd"=w1445:bool, "status"=w1446:string)
                                n577 = local write "ConnectArray"(w1447) -> ()
                                n578 = local write "TCPconnecCmd"(w1445) -> ()
                                n579 = local write "Status"(w1446) -> ()
                              }
                              frame #1 {
                                n580 = Wait (ms)(milliseconds to wait=u32 1000) -> ()  [unwired: 1 out]
                              }
                              frame #2 {
                                n581 = Tick Count (ms)() -> (millisecond timer value=w1454:u32)
                                n582 = while {
                                tunnel: w1454 -> [w1458]
                                tunnel: [w1455] -> w1453
                                i -> [w1467]
                                stop <- w1460 stop-if-true
                                n583 = Tick Count (ms)() -> (millisecond timer value=w1459:u32)
                                n584 = Subtract(x=w1459, y=w1458) -> (x-y=w1457:u32)
                                n585 = local read "MoveInProgress"() -> (w1462:bool)
                                n586 = Greater?(x=w1457, y=u32 10000) -> (0:w1455:bool)
                                n587 = local read "RunON/OFF"() -> (w1464:bool)
                                n588 = local read "restart"() -> (w1465:bool)
                                n589 = local read "stop"() -> (w1466:bool)
                                n590 = Wait (ms)(milliseconds to wait=u32 100) -> ()  [unwired: 1 out]
                                n591 = Not(x=w1462) -> (.not. x?=w1461:bool)
                                n592 = Not(x=w1464) -> (.not. x?=w1463:bool)
                                n593 = Compound Arithmetic op=OR(w1461, w1466, w1465, w1463, w1455) -> (w1460:bool)
                                "# loops waiting 4 move" <- w1467
                                }
                                "MoveInProgress 2" <- w1453
                              }
                            }
                          }
                        }
                        n594 = Index Array(array=w1410) -> (element #1=→"element":string, element #2=→"element 2":string, element #3=→"element 3":string, element #4=→"element 4":string, element #5=→"element 5":string, element #6=→"element 6":string, element #7=→"element 7":string, element #8=→"element 8":string, element #9=→"element 9":string)  [unwired: 9 in]
                        n595 = local write "State"(11) -> ()
                      }
                      frame #14 {
                        # "Statistics"
                        n596 = local read "Beam Detected"() -> (w1469:bool)
                        n597 = case shown="False" w1469 {
                          tunnel: w1471 -> [_ w1482]
                          tunnel: w1470 -> [_ w1481]
                          frame False {
                          }
                          frame True {
                            # "Save history"
                            n598 = local read "History XY Buffer"() -> (w1480:T14)
                            n599 = local read "Main processing loop i"() -> (w1478:i32)
                            n600 = Index Array(array=w1480, index (row)=w1481) -> (element=w1473:T17)  [unwired: 1 in]
                            n601 = Unbundle By Name(w1482) -> ("Center"=w1479:cluster{"X":sgl, "Y":sgl})
                            n602 = Equal To 0?(x=w1478) -> (x = 0?=w1477:bool)
                            n603 = call "Add point in History v2.vi"("History XY In"=w1473, "New Point"=w1479, "clear first (no:F)"=w1477, "chart length (points)"="History # of points") -> ("History XY Out"=w1474:T17)  [unwired: 4 in]
                            n604 = local read "History XY Buffer"() -> (w1475:T14)
                            n605 = call "Add Or Replace History Array.vi"("History XY Buffer In"=w1475, "History XY In"=w1474, "Index"=w1481, "# of points"="History # of points") -> ("History XY Buffer Out"=w1476:T14)  [unwired: 6 in]
                            n606 = local write "History XY Buffer"(w1476) -> ()
                          }
                        }
                      }
                      frame #15 {
                        # "Statistics"
                        n607 = local read "NewAvg"() -> (w1484:bool)
                        n608 = case shown="False" w1484 {
                          tunnel: w1483 -> [_ w1485]
                          frame False {
                          }
                          frame True {
                            # "Save data in buffers to display"
                            n609 = local read "ImgData Avg"() -> (w1493:T23)
                            n610 = local read "Centroid Avg Buffer"() -> (w1488:cluster{"X Centroid":sgl, "Y Centroid":sgl}[])
                            n611 = Unbundle By Name(w1493) -> ("Centroid Avg"=w1492:cluster{"X":sgl, "Y":sgl})
                            n612 = call-poly "Replace Or Add.vi"("Coord"=w1492, "Index"=w1485, "Coord Array In"=w1488) -> ("Coord Array Out"=w1486:cluster{"X":sgl, "Y":sgl}[])  [unwired: 8 in]
                            n613 = local write "Centroid Avg Buffer"(w1486) -> ()
                            n614 = local read "Avg Img Buffer"() -> (w1489:u8[][][])
                            n615 = local read "Avg Img"() -> (w1487:T1)
                            n616 = call "IMAQ ImageToArray"("Image"=w1487) -> ("Image Pixels (U8)"=w1491:u8[][])  [unwired: 2 in, 5 out]
                            n617 = call-poly "Replace Or Add.vi"("Img"=w1491, "Index"=w1485, "Img Array In"=w1489) -> ("Img Array Out"=w1490:u8[][][])  [unwired: 8 in]
                            n618 = local write "Avg Img Buffer"(w1490) -> ()
                          }
                        }
                      }
                      frame #16 {
                        # "Choose image to display"
                        n619 = local read "USB/RS170 cams"() -> (w1497:bool)
                        n620 = local read "Fancy Display Options"() -> (w1508:T24)
                        n621 = local read "Output Img"() -> (w1514:T1)
                        n622 = local read "Display"() -> (w1503:T26)
                        n623 = local read "Thresh Img"() -> (w1511:T1)
                        n624 = local read "Avg Img"() -> (w1512:T1)
                        n625 = local read "Displayed Image"() -> (w1496:u8[][])
                        n626 = Unbundle By Name(w1503) -> ("Show Best Rect"=w1502:bool)
                        n627 = Build Array(w1514, w1512, w1511) -> (w1510:T1[])
                        n628 = Unbundle By Name(w1508) -> ("Use fancy display"=w1507:bool, "show acquired image"=w1506:bool, "Show Edges"=w1505:bool, "Show Full Ellipse"=w1501:bool, "Show Ellipses points"=w1504:bool)
                        n629 = Select(t=0.8, s=w1497, f=1.0) -> (s? t:f=w1500:dbl)
                        n630 = Array Size(array=w1496) -> (size(s)=→"size(s)":i32[])
                        n631 = Index Array(array=w1510, index="Image Selector") -> (element=w1509:T1)
                        n632 = local write "State"(6) -> ()
                        n633 = call "IMAQ ImageToArray"("Image"=w1509) -> ("Image Pixels (U8)"=w1494:u8[][])  [unwired: 2 in, 5 out]
                        "Displayed Image" <- w1494
                        n634 = property on="Fancy Display" class="Pict"("ZoomFactor"=w1500) -> ()  [unwired: 2 in, 2 out]
                        n635 = case shown="True" w1507 {
                          tunnel: w1494 -> [_ w1524]
                          tunnel: w1506 -> [_ w1538]
                          tunnel: w1505 -> [_ w1537]
                          tunnel: w1504 -> [_ w1536]
                          tunnel: w1502 -> [_ w1522]
                          tunnel: w1501 -> [_ w1526]
                          frame False {
                          }
                          frame True {
                            n636 = local read "Fancy Display"() -> (w1520:picture)
                            n637 = call <vilib>:"Flatten Pixmap.vi"("8-bit pixmap"=w1524) -> ("image data"=w1540:T44)  [unwired: 10 in]
                            n638 = call <vilib>:"Draw Rect.vi"("picture"=w1520, "rect"=T32 {"left"=0, "top"=0, "right"=800, "bottom"=600}, "fill?(F)"=TRUE, "color(black)"=u32 16777226) -> ("new picture"=w1517:picture)  [unwired: 5 in]
                            n639 = local read "Beam Detected"() -> (w1523:bool)
                            n640 = call <vilib>:"Draw Flattened Pixmap.vi"("image data"=w1540, "picture"=w1517) -> ("new picture"=w1539:picture)  [unwired: 7 in]
                            n641 = local read "RectFilter"() -> (w1532:T13)
                            n642 = Select(t=w1539, s=w1538, f=w1517) -> (s? t:f=w1534:picture)
                            n643 = Unbundle By Name(w1532) -> ("Left"=w1531:i32, "Top"=w1530:i32, "Right"=w1529:i32, "Bottom"=w1528:i32)
                            n644 = And(x=w1523, y=w1522) -> (x .and. y?=w1521:bool)
                            n645 = Bundle("Left"=w1531, "Top"=w1530, "Right"=w1529, "Bottom"=w1528) -> (w1527:T45)  [unwired: 1 in]
                            n646 = case shown="True" w1521 {
                              tunnel: w1534 -> [w1545 w1550]
                              tunnel: [w1545 w1549] -> w1533
                              tunnel: w1527 -> [_ w1548]
                              frame False {
                              }
                              frame True {
                                n647 = call <vilib>:"Draw Rect.vi"("picture"=w1550, "rect"=w1548, "color(black)"=u32 16323327, "pen"=T33 {"Width"=2, "Style"=enum."Solid"}) -> ("new picture"=w1549:picture)  [unwired: 5 in]
                              }
                            }
                            n648 = case shown="True" w1537 {
                              tunnel: w1533 -> [w1566 w1568]
                              tunnel: [w1566 w1567] -> w1535
                              frame False {
                              }
                              frame True {
                                n649 = local read "Ellipse edges"() -> (w1570:cluster{"X":sgl, "Y":sgl}[])
                                n650 = Index Array(array=w1570, index=0) -> (element=w1569:cluster{"X":sgl, "Y":sgl})
                                n651 = call <vilib>:"Move Pen.vi"("new position"=w1569, "picture"=w1568) -> ("new picture"=w1572:picture)  [unwired: 3 in]
                                n652 = for {
                                tunnel: w1570 -> [w1576] mode=indexing
                                shift-right: [w1574] -> w1567
                                shift-left: w1572 -> [w1573]
                                n653 = call <vilib>:"Draw Line.vi"("picture"=w1573, "end point"=w1576, "color(black)"=u32 4390888, "pen"=T34 {"Width"=4, "Style"=enum."Solid"}) -> ("new picture"=w1574:picture)  [unwired: 5 in]
                                }
                              }
                            }
                            n654 = case shown="True" w1536 {
                              tunnel: w1535 -> [w1551 w1553]
                              tunnel: [w1551 w1552] -> w1525
                              frame False {
                              }
                              frame True {
                                w1560 = T34 {"Width"=10, "Style"=enum."Solid"} ("pen")
                                w1561 = u32 3473194 ("color(black)")
                                n655 = local read "Ellipse"() -> (w1554:T10)
                                n656 = Unbundle By Name(w1554) -> ("Major Axis.Point 1"=w1558:cluster{"X":sgl, "Y":sgl})
                                n657 = Unbundle By Name(w1554) -> ("Major Axis.Point 2"=w1557:cluster{"X":sgl, "Y":sgl})
                                n658 = Unbundle By Name(w1554) -> ("Center"=w1559:cluster{"X":sgl, "Y":sgl})
                                n659 = Unbundle By Name(w1554) -> ("Minor Axis.Point 1"=w1556:cluster{"X":sgl, "Y":sgl})
                                n660 = Unbundle By Name(w1554) -> ("Minor Axis.Point 2"=w1555:cluster{"X":sgl, "Y":sgl})
                                n661 = call <vilib>:"Draw Point.vi"("picture"=w1553, "point(x,y)"=w1559, "color(black)"=w1561, "pen"=w1560) -> ("new picture"=w1565:picture)  [unwired: 5 in]
                                n662 = call <vilib>:"Draw Point.vi"("picture"=w1565, "point(x,y)"=w1558, "color(black)"=w1561, "pen"=w1560) -> ("new picture"=w1564:picture)  [unwired: 5 in]
                                n663 = call <vilib>:"Draw Point.vi"("picture"=w1564, "point(x,y)"=w1557, "color(black)"=w1561, "pen"=w1560) -> ("new picture"=w1563:picture)  [unwired: 5 in]
                                n664 = call <vilib>:"Draw Point.vi"("picture"=w1563, "point(x,y)"=w1556, "color(black)"=w1561, "pen"=w1560) -> ("new picture"=w1562:picture)  [unwired: 5 in]
                                n665 = call <vilib>:"Draw Point.vi"("picture"=w1562, "point(x,y)"=w1555, "color(black)"=w1561, "pen"=w1560) -> ("new picture"=w1552:picture)  [unwired: 5 in]
                              }
                            }
                            n666 = case shown="True" w1526 {
                              tunnel: w1525 -> [w1541 w1543]
                              frame False {
                                n667 = local write "Fancy Display"(w1541) -> ()
                              }
                              frame True {
                                n668 = local read "Ellipse"() -> (w1542:T10)
                                n669 = call "Draw Ellipse.vi"("picture"=w1543, "Ellipse"=w1542) -> ("new picture"=w1544:picture)  [unwired: 9 in]
                                n670 = local write "Fancy Display"(w1544) -> ()
                              }
                            }
                          }
                        }
                      }
                      frame #17 {
                        n671 = local read "LoopMode"() -> (w1580:bool)
                        n672 = case shown="False" w1580 {
                          tunnel: w1578 -> [w1581 _]
                          frame False {
                            # "Display croos hairs of Detection ROI"
                            # "Accumulate statistics on whether beam centroid  is within specified range of target"
                            n673 = local read "ImgData Avg"() -> (w1598:T23)
                            n674 = Unbundle By Name("Target Area  Display") -> ("Show Target Reached"=w1600:bool)
                            n675 = Unbundle By Name("Target Area  Display") -> ("Show Init Correction"=w1599:bool)
                            n676 = Unbundle By Name("Target Area  Display") -> ("Show Variance"=w1601:bool)
                            n677 = local read "ImgDataArray"() -> (w1597:T15)
                            n678 = Unbundle By Name(w1598) -> ("Centroid Avg"=w1596:cluster{"X":sgl, "Y":sgl})
                            n679 = for {
                              tunnel: w1597 -> [w1635] mode=indexing
                              tunnel: [w1638] -> w1628 mode=indexing
                              tunnel: [w1637] -> w1627 mode=indexing
                              tunnel: w1596 -> [w1633]
                              n680 = Unbundle By Name(w1635) -> ("Center"=w1634:cluster{"X":sgl, "Y":sgl})
                              n681 = Subtract(x=w1634, y=w1633) -> (x-y=w1636:cluster{"X":sgl, "Y":sgl})
                              n682 = Absolute Value(x=w1636) -> (abs(x)=w1632:cluster{"X":sgl, "Y":sgl})
                              n683 = Unbundle(w1632) -> ("X"=w1638:sgl, "Y"=w1637:sgl)
                            }
                            n684 = Select(t=u32 16711680 ("Color"), s=w1601, f=u32 16777216 ("Color")) -> (s? t:f=w1613:u32)
                            n685 = Select(t=u32 16776704 ("Color"), s=w1600, f=u32 16777216 ("Color")) -> (s? t:f=w1606:u32)
                            n686 = Select(t=u32 3381759 ("Color"), s=w1599, f=u32 16777216 ("Color")) -> (s? t:f=w1617:u32)
                            n687 = property on="Target Area" class="XYGraph (strict)"("Active Plot"=u32 1, "Plot.Fill/Pt. Color"=w1606) -> ()  [unwired: 2 in, 2 out]
                            n688 = property on="Target Area" class="XYGraph (strict)"("Active Plot"=u32 0, "Plot.Plot Color"=w1613) -> ()  [unwired: 2 in, 2 out]
                            n689 = property on="Target Area" class="XYGraph (strict)"("Active Plot"=u32 2, "Plot.Plot Color"=w1617) -> ()  [unwired: 2 in, 2 out]
                            n690 = local read "Region of Interest"() -> (w1582:i32[])
                            n691 = call <vilib>:"Std Deviation and Variance.vi"("X"=w1628) -> ("mean"=w1609:dbl)  [unwired: 1 in, 2 out]
                            n692 = call <vilib>:"Std Deviation and Variance.vi"("X"=w1627) -> ("mean"=w1608:dbl)  [unwired: 1 in, 2 out]
                            n693 = Bundle("mean"=w1609, "mean"=w1608) -> (w1595:cluster{"mean":dbl, "mean":dbl})  [unwired: 1 out]
                            "Avg Variation" <- w1595
                            n694 = local read "DeviationArray"() -> (w1626:cluster{"X Centroid":sgl, "Y Centroid":sgl}[])
                            n695 = call-poly "Add ROI Offset.vi"("Region of Interest"=w1582, "RectFilter In"=w1581) -> ("RectFilter Out"=w1583:T13)  [unwired: 3 in]
                            n696 = Unbundle By Name(w1583) -> ("Left"=w1589:i32, "Top"=w1588:i32, "Right"=w1586:i32, "Bottom"=w1585:i32)
                            n697 = for {
                              tunnel: w1626 -> [w1631] mode=indexing
                              tunnel: [w1630] -> w1625 mode=indexing
                              tunnel: [w1629] -> w1624 mode=indexing
                              n698 = Unbundle(w1631) -> ("X Centroid"=w1630:sgl, "Y Centroid"=w1629:sgl)
                            }
                            n699 = local read "Deviation"() -> (w1607:cluster{"Dev. X":sgl, "Dev. Y":sgl})
                            n700 = Divide(x="Initiate Correction Range", y=sgl 100.0) -> (x/y=w1594:sgl)
                            n701 = call "ellipse graph.vi"("# of points"=100, "Avg Variation"=w1595, "Center"=w1607) -> ("ellipse graph"=w1618:cluster{dbl[], dbl[]})  [unwired: 1 in, 5 out]
                            n702 = Bundle("Right"=w1586, "Bottom"=w1585) -> (w1584:cluster{"Right":i32, "Bottom":i32})  [unwired: 1 in]
                            n703 = Bundle("Left"=w1589, "Top"=w1588) -> (w1587:cluster{"Left":i32, "Top":i32})  [unwired: 1 in]
                            n704 = call "circle graph.vi"("# of points"=100, "Radius"=w1594) -> ("circle graph"=w1592:cluster{dbl[], dbl[]})  [unwired: 7 out]
                            n705 = Bundle(w1625, w1624) -> (w1620:cluster{sgl[], sgl[]})  [unwired: 1 out]
                            n706 = Build Array(w1592, w1620, w1618) -> (→"Target Area":cluster{dbl[], dbl[]}[])
                            n707 = property on="Displayed Image" class="IntGraph (strict)"("Active Cursor"=u32 6, "Cursor.Cursor Position"=w1587, "Active Cursor"=u32 7, "Cursor.Cursor Position"=w1584) -> ()  [unwired: 2 in, 2 out]
                          }
                          frame True {
                          }
                        }
                        n708 = local write "State"(8) -> ()
                      }
                      frame #18 {
                        # "Target Area"
                        # "overlay cross-hairs on image at centroid and target locations"
                        # "X and Y profile"
                        # "Display"
                        # "cursor position"
                        # "target"
                        # "centroid avg"
                        n709 = local read "Display Current"() -> (w1662:bool)
                        n710 = case shown="True" w1662 {
                          tunnel: [w1715 w1722] -> w1694
                          tunnel: [w1719 w1721] -> w1658
                          tunnel: [w1716 w1720] -> w1679
                          tunnel: w1657 -> [w1718 _]
                          frame False {
                            n711 = local read "Image Selector"() -> (w1719:u16)
                            n712 = Index Array(array=w1718, index=w1719) -> (element=w1717:T36)
                            n713 = Unbundle By Name(w1717) -> ("CorrectConfig Cluster.Target"=w1716:cluster{"X Target":sgl, "Y Target":sgl}, "CorrectConfig Cluster.Region of Interest"=w1715:i32[])
                          }
                          frame True {
                            n714 = local read "USB cameras Indic"() -> (w1721:i32)
                            n715 = local read "Region of Interest"() -> (w1722:i32[])
                            n716 = local read "Target"() -> (w1720:cluster{"X Target":sgl, "Y Target":sgl})
                          }
                        }
                        n717 = local read "Centroid Avg Buffer"() -> (w1672:cluster{"X Centroid":sgl, "Y Centroid":sgl}[])
                        n718 = local read "History XY Buffer"() -> (w1641:T14)
                        n719 = local read "Img Size"() -> (w1661:i32[])
                        n720 = Not Equal?(x=w1694, y=i32[] [0, 0, 0, 0] ("Region of Interest")) -> (x != y?=w1660:bool)
                        n721 = Index Array(array=w1641, index (col)=0 ("disabled index (col)")) -> (element=→"history last shots":T17)  [unwired: 1 in]
                        n722 = Select(t=w1694, s=w1660, f=w1661) -> (s? t:f=w1659:i32[])
                        n723 = property on="Displayed Image" class="IntGraph (strict)"("Active Cursor"=u32 0) -> ("Cursor.Cursor Position"=w1692:T40)  [unwired: 2 in, 2 out]
                        n724 = property on="Displayed Image" class="IntGraph (strict)"("Active Cursor"=u32 1, "Cursor.Cursor Position"=w1679) -> ()  [unwired: 2 in, 2 out]
                        n725 = Index Array(array=w1672, index=w1658) -> (element=w1663:cluster{"X Centroid":sgl, "Y Centroid":sgl})
                        n726 = case shown="True" "set scales" {
                          tunnel: w1659 -> [_ w1708]
                          frame False {
                          }
                          frame True {
                            n727 = for {
                              tunnel: w1708 -> [w1709] mode=indexing
                              i -> [w1710]
                              # "set scales"
                              n728 = case shown="3" w1710 {
                                tunnel: w1709 -> [w1711 w1712 w1713 w1714 _]
                                frame 0 {
                                n729 = property on="Displayed Image" class="IntGraph (strict)"("XScale.Offset"=w1711, "XScale.Minimum"=w1711) -> ()  [unwired: 2 in, 2 out]
                                n730 = property on="X Intensity" class="WFGraph (strict)"("XScale.Offset"=w1711, "XScale.Minimum"=w1711) -> ()  [unwired: 2 in, 2 out]
                                }
                                frame 1 {
                                n731 = property on="Displayed Image" class="IntGraph (strict)"("YScale.Offset"=w1712, "YScale.Minimum"=w1712) -> ()  [unwired: 2 in, 2 out]
                                n732 = property on="Y Intensity" class="WFGraph (strict)"("XScale.Offset"=w1712, "XScale.Minimum"=w1712) -> ()  [unwired: 2 in, 2 out]
                                }
                                frame 2 {
                                n733 = property on="Displayed Image" class="IntGraph (strict)"("XScale.Maximum"=w1713) -> ()  [unwired: 2 in, 2 out]
                                n734 = property on="X Intensity" class="WFGraph (strict)"("XScale.Maximum"=w1713) -> ()  [unwired: 2 in, 2 out]
                                }
                                frame 3 {
                                n735 = property on="Displayed Image" class="IntGraph (strict)"("YScale.Maximum"=w1714) -> ()  [unwired: 2 in, 2 out]
                                n736 = property on="Y Intensity" class="WFGraph (strict)"("XScale.Maximum"=w1714) -> ()  [unwired: 2 in, 2 out]
                                }
                                frame 4, Default {
                                }
                              }
                            }
                          }
                        }
                        n737 = for {
                          tunnel: w1641 -> [w1703] mode=indexing
                          tunnel: [w1698] -> _ mode=indexing
                          tunnel: [w1697] -> _ mode=indexing
                          tunnel: [w1696] -> w1651 mode=indexing
                          n738 = call "History remove zeros.vi"("History XY In"=w1703) -> ("History XY Out"=w1702:T17)  [unwired: 2 in]
                          n739 = for {
                            tunnel: w1702 -> [w1707] mode=indexing
                            tunnel: [w1706] -> w1700 mode=indexing
                            tunnel: [w1705] -> w1701 mode=indexing
                            tunnel: [w1704] -> w1699 mode=indexing
                            n740 = Unbundle(w1707) -> ("seconds since 1Jan1904"=w1706:timestamp, "number: 0 to 1"=w1705:dbl, "number: 0 to 1"=w1704:dbl)
                          }
                          n741 = Bundle(w1700, w1701) -> (w1698:cluster{timestamp[], dbl[]})  [unwired: 1 in]
                          n742 = Bundle(w1700, w1699) -> (w1697:cluster{timestamp[], dbl[]})  [unwired: 1 in]
                          n743 = Build Array(w1698, w1697) -> (w1696:cluster{timestamp[], dbl[]}[])
                        }
                        n744 = local read "Initiate Correction Range"() -> (w1665:i16)
                        n745 = property on="Displayed Image" class="IntGraph (strict)"("Active Cursor"=u32 2, "Cursor.Cursor Position"=w1663) -> ()  [unwired: 2 in, 2 out]
                        n746 = Unbundle By Name(w1692) -> ("Cursor Y"=w1691:dbl, "Cursor X"=w1688:dbl)
                        n747 = Index Array(array=w1694, index #1=0 ("index"), index #2=1 ("index")) -> (element #1=w1681:i32, element #2=w1680:i32)
                        n748 = Unbundle By Name(w1679) -> ("X Target"=w1675:sgl, "Y Target"=w1674:sgl)
                        n749 = local read "Displayed Image"() -> (w1654:u8[][])
                        n750 = Subtract(x=w1688, y=w1681) -> (x-y=w1684:dbl)
                        n751 = Subtract(x=w1691, y=w1680) -> (x-y=w1685:dbl)
                        n752 = Divide(x=w1665, y=sgl 100.0) -> (x/y=w1666:sgl)
                        n753 = local read "History XY Buffer"() -> (w1652:T14)
                        n754 = Multiply(x=w1663, y=w1666) -> (x*y=w1671:cluster{"X Centroid":sgl, "Y Centroid":sgl})
                        n755 = property on="History Display" class="XYGraph (strict)"("Active Cursor"=u32 0, "Cursor.Cursor Y"=w1675, "Active Cursor"=u32 1, "Cursor.Cursor Y"=w1674) -> ()  [unwired: 2 in, 2 out]
                        n756 = Index Array(array=w1651) -> (element #1=→"History Display 2":cluster{timestamp[], dbl[]}[], element #2=→"History Display 3":cluster{timestamp[], dbl[]}[], element #3=→"History Display 4":cluster{timestamp[], dbl[]}[], element #4=→"History Display 5":cluster{timestamp[], dbl[]}[], element #5=→"History Display 6":cluster{timestamp[], dbl[]}[], element #6=→"History Display 7":cluster{timestamp[], dbl[]}[], element #7=→"History Display 8":cluster{timestamp[], dbl[]}[], element #8=→"History Display 9":cluster{timestamp[], dbl[]}[], element #9=→"History Display 10":cluster{timestamp[], dbl[]}[])  [unwired: 18 in]
                        n757 = Index Array(array=w1654, index (row)=w1685) -> (element=→"X Intensity":u8[])  [unwired: 1 in]
                        n758 = Delete From Array(array=w1654, length=1, index (col)=w1684) -> (deleted portion=w1687:u8[][])  [unwired: 1 in, 1 out]
                        n759 = call "Rectangle Overlay for 2 Cursors.vi"("Radius"=w1671, "Coord"=w1679) -> ("Right Bottom"=w1669:cluster{dbl, dbl}, "Left Top"=w1670:cluster{dbl, dbl})  [unwired: 2 in, 6 out]
                        n760 = Transpose 2D Array(2D array=w1687) -> (transposed array=→"Y Intensity":u8[][])
                        n761 = Index Array(array=w1652, index (row)=w1658) -> (element=w1656:T17)  [unwired: 1 in]
                        n762 = call "History remove zeros.vi"("History XY In"=w1656) -> ("History XY Out"=→"History Display":T17)  [unwired: 2 in]
                        n763 = property on="Displayed Image" class="IntGraph (strict)"("Active Cursor"=u32 4, "Cursor.Cursor Position"=w1670, "Active Cursor"=u32 5, "Cursor.Cursor Position"=w1669) -> ()  [unwired: 2 in, 2 out]
                      }
                      frame #19 {
                        n764 = local read "MoveInProgressTimeIN"() -> (w1730:u32)
                        n765 = local read "LoopMode"() -> (w1738:bool)
                        n766 = local read "NewAvg"() -> (w1735:bool)
                        n767 = local read "start"() -> (w1732:u32)
                        n768 = Tick Count (ms)() -> (millisecond timer value=w1731:u32)
                        n769 = Wait (ms)(milliseconds to wait="milliseconds to wait") -> ()  [unwired: 1 out]
                        n770 = Subtract(x=w1731, y=w1732) -> (x-y=→"one loop":u32)
                        n771 = case shown="True" w1738 {
                          tunnel: [w1759 w1773] -> w1734
                          tunnel: w1726 -> [w1756 w1771]
                          tunnel: w1723 -> [w1749 w1762]
                          frame False {
                            # "Manual mode"
                            n772 = local read "Auto Detect Param"() -> (w1753:bool)
                            n773 = local read "error CamS"() -> (w1760:errorcluster)
                            n774 = local read "RunON/OFF"() -> (w1761:bool)
                            n775 = Greater Or Equal?(x=w1756, y=20) -> (x >= y?=w1752:bool)
                            n776 = Implies(1:w1752, 2:w1753) -> (0:w1751:bool)
                            n777 = Unbundle By Name(w1760) -> ("status"=w1757:bool)
                            n778 = Not(x=w1751) -> (.not. x?=w1750:bool)
                            n779 = Not(x=w1761) -> (.not. x?=w1758:bool)
                            n780 = local write "Auto Detect Param"(w1750) -> ()
                            n781 = And(x=w1753, y=w1752) -> (x .and. y?=w1754:bool)
                            n782 = Compound Arithmetic op=OR(w1749, w1758, w1757, w1754) -> (w1759:bool)
                          }
                          frame True {
                            # "Automatic mode"
                            n783 = local read "OpenTime"() -> (w1766:u32)
                            n784 = local read "# imgs to avg"() -> (w1772:i32)
                            n785 = Tick Count (ms)() -> (millisecond timer value=w1767:u32)
                            n786 = Subtract(x=w1767, y=w1766) -> (x-y=w1765:u32)
                            n787 = local read "NewAvg"() -> (w1774:bool)
                            n788 = Multiply(x=w1772, y=10) -> (x*y=w1770:i32)
                            n789 = Greater?(x=w1765, y="Auto Time Out (ms)") -> (0:w1764:bool)
                            n790 = Greater?(x=w1771, y=w1770) -> (0:w1769:bool)
                            n791 = Compound Arithmetic op=OR(w1762, w1774, w1769, w1764) -> (w1773:bool)
                          }
                        }
                        n792 = case shown="True" w1735 {
                          frame False {
                          }
                          frame True {
                            # "re-intialize for new average"
                            n793 = Initialize Array(T30 {"X Intensity"=[], "Y Intensity"=[], "Max Intensity"=0, "Center"={"X"=0, "Y"=0}, "Radius"={"Rx"=0, "Ry"=0}} ("ImgData"), 0 ("dimension size")) -> (w1747:T37)
                            n794 = Initialize Array(cluster{"Width (x)":sgl, "Height (y)":sgl} {"Width (x)"=0.0, "Height (y)"=0.0} ("SpotSizeAvg"), 0 ("dimension size")) -> (w1744:cluster{"Width (x)":sgl, "Height (y)":sgl}[])
                            n795 = local write "ImgDataArray"(w1747) -> ()
                            n796 = local write "DeviationArray"(w1744) -> ()
                          }
                        }
                        n797 = Subtract(x=w1731, y=w1730) -> (x-y=w1729:u32)
                        n798 = Greater?(x=w1729, y=u32 10000) -> (0:w1727:bool)
                        n799 = case shown="True" w1727 {
                          frame False {
                          }
                          frame True {
                            # "reset InProgress if  stuck for more \nthan 10s."
                            n800 = Initialize Array("", 0 ("dimension size")) -> (w1742:string[])
                            n801 = local write "InProgress"(w1742) -> ()
                          }
                        }
                        n802 = case shown="True" w1734 {
                          tunnel: w1737 -> [_ w1778]
                          tunnel: w1725 -> [w1775 w1777]
                          tunnel: [w1775 w1776] -> w1724
                          frame False {
                          }
                          frame True {
                            n803 = stacked-sequence {
                              tunnel: w1778 -> [w1785 _]
                              tunnel: w1777 -> [w1799 _]
                              tunnel: [w1782 _] -> w1776
                              frame #0 {
                                # "save data"
                                n804 = local read "Acquisition Parameters"() -> (w1787:T27)
                                n805 = local read "Acquisition Parameters dx"() -> (w1788:T11)
                                n806 = local read "Correction Parameters"() -> (w1798:cluster{"X":sgl, "Y":sgl, "Movement Type":u16})
                                n807 = local read "Background Path"() -> (w1791:path)
                                n808 = local read "Detection Parameters"() -> (w1794:T21)
                                n809 = local read "USB/RS170 cams"() -> (w1786:bool)
                                n810 = local read "X calibration"() -> (w1781:cluster{dbl, dbl}[])
                                n811 = local read "Y calibration"() -> (w1780:cluster{dbl, dbl}[])
                                n812 = local read "Region of Interest"() -> (w1797:i32[])
                                n813 = local read "Reference Path"() -> (w1790:path)
                                n814 = local read "Target"() -> (w1796:cluster{"X Target":sgl, "Y Target":sgl})
                                n815 = local read "Reverse"() -> (w1795:cluster{"Reverse X":bool, "Reverse Y":bool})
                                n816 = case shown="True" FALSE {
                                tunnel: w1785 -> [_ w1800]
                                frame False {
                                }
                                frame True {
                                n817 = local read "Feedback"() -> (w1801:bool)
                                n818 = local read "Corr"() -> (w1803:bool[])
                                n819 = Replace Array Subset(array=w1803, new element=w1801, index=w1800) -> (w1802:bool[])
                                n820 = local write "Corr"(w1802) -> ()
                                }
                                }
                                n821 = Index Array(array=w1799, index=w1785) -> (element=w1793:T36)
                                n822 = Select(t=w1788, s=w1786, f=w1787) -> (s? t:f=w1789:T27)
                                n823 = local read "Mirrors"() -> (w1784:u8[])
                                n824 = Bundle By Name(cluster=w1793, "CorrectConfig Cluster.Detection Parameters"=w1794, "CorrectConfig Cluster.Reverse"=w1795, "CorrectConfig Cluster.Target"=w1796, "CorrectConfig Cluster.Region of Interest"=w1797, "CorrectConfig Cluster.Correction Parameters"=w1798, "CorrectConfig Cluster.Acquisition Parameters"=w1789, "CorrectConfig Cluster.Background Path"=w1791, "CorrectConfig Cluster.Reference Path"=w1790, "CorrectConfig Cluster.XCalibration"=w1781, "CorrectConfig Cluster.YCalibration"=w1780) -> (w1792:T36)
                                n825 = Replace Array Subset(array=w1799, new element=w1792, index=w1785) -> (w1783:T9)
                                n826 = for {
                                tunnel: w1784 -> [w1808] mode=indexing
                                tunnel: w1783 -> [w1807] mode=indexing
                                tunnel: [w1804] -> w1782 mode=indexing
                                n827 = local read "DeviceList"() -> (w1809:T16)
                                n828 = call "NumberToDeviceID-v2.vi"("device raw"=w1808, "DeviceList"=w1809) -> ("DeviceID"=w1805:T31, "Name"=w1806:string)  [unwired: 5 in, 3 out]
                                n829 = Bundle By Name(cluster=w1807, "Name"=w1806, "DeviceID"=w1805) -> (w1804:T36)
                                }
                              }
                              frame #1 {
                                # "Dispose buffer"
                                n830 = local read "Img Buffer"() -> (w1812:T1[])
                                n831 = local read "error CamS"() -> (w1811:errorcluster)
                                n832 = local read "OpenTime"() -> (w1815:u32)
                                n833 = Tick Count (ms)() -> (millisecond timer value=w1813:u32)
                                "Switch in" <- w1813
                                n834 = call "IMAQ Dispose Buffer.vi"("error in"=w1811, "Img Buffer In"=w1812) -> ("error out"=w1810:errorcluster)  [unwired: 1 in]
                                n835 = Subtract(x=w1813, y=w1815) -> (x-y=→"AcqTime":u32)
                                n836 = local write "error CamS"(w1810) -> ()
                                n837 = local write "CloseCam"(TRUE ("CloseCam")) -> ()
                              }
                            }
                          }
                        }
                        n838 = local write "State"(12) -> ()
                      }
                    }
                    "Main processing loop i" <- w842
                  }
                  n839 = local write "CamConfigArray"(w834) -> ()
                }
              }
            }
            n840 = for {
              tunnel: w427 -> [w582] mode=indexing
              tunnel: [w581] -> w425 mode=indexing
              tunnel: [w580] -> w424 mode=indexing
              n841 = Unbundle By Name(w582) -> ("ImageServer"=w583:cluster{"IPAddress":string, "Port":i32})
              n842 = Unbundle By Name(w583) -> ("IPAddress"=w581:string, "Port"=w580:i32)
            }
            "Image IPs" <- w425
            "Image Ports" <- w424
            n843 = while {
              tunnel: w429 -> [w584]
              stop <- w585 stop-if-true
              n844 = local read "restart"() -> (w585:bool)
              n845 = event shown="[20] \"Grab reference Image\": Mouse Up" {
                selector: _ -> [_ _ _ _ _ _ _ _ _ _ _ _ _ _ _ _ _ _ _ _ _ _ _]
                dyn-events: _ -> [_ _ _ _ _ _ _ _ _ _ _ _ _ _ _ _ _ _ _ _ _ _ _]
                timeout: 500 -> [_ _ _ _ _ _ _ _ _ _ _ _ _ _ _ _ _ _ _ _ _ _ _]
                tunnel: w584 -> [_ _ _ _ _ _ _ w666 _ _ _ _ _ _ _ _ _ _ _ _ _ _ _]
                event Timeout {
                  n846 = event-data() -> ()  [unwired: 3 out]
                }
                event "MoveInProgress": Value Change {
                  n847 = event-data() -> ("OldVal"=w588:bool, "NewVal"=w587:bool)  [unwired: 1 out]
                  n848 = Not(x=w588) -> (.not. x?=w589:bool)
                  n849 = And(x=w589, y=w587) -> (x .and. y?=w590:bool)
                  n850 = case shown="False" w590 {
                    frame False {
                    }
                    frame True {
                      n851 = Tick Count (ms)() -> (millisecond timer value=→"MoveInProgressTimeIN":u32)
                    }
                  }
                }
                event "Calibrate": Value Change {
                  n852 = event-data() -> ("NewVal"=w592:bool)  [unwired: 2 out]
                  n853 = case shown="False" w592 {
                    frame False {
                      n854 = local read "X calibration"() -> (w605:cluster{dbl, dbl}[])
                      n855 = local read "Y calibration"() -> (w609:cluster{dbl, dbl}[])
                      n856 = Array Size(array=w605) -> (size(s)=w607:i32)
                      n857 = Array Size(array=w609) -> (size(s)=w611:i32)
                      n858 = for {
                        tunnel: w609 -> [w624] mode=indexing
                        tunnel: w605 -> [w623] mode=indexing
                        tunnel: [w622] -> w595 mode=indexing
                        tunnel: [w621] -> w603 mode=indexing
                        tunnel: [w620] -> w596 mode=indexing
                        tunnel: [w619] -> w599 mode=indexing
                        n859 = Unbundle(w623) -> (w622:dbl, w621:dbl)
                        n860 = Unbundle(w624) -> (w620:dbl, w619:dbl)
                      }
                      n861 = Decrement(x=w607) -> (x-1=w608:i32)
                      n862 = Decrement(x=w611) -> (x-1=w612:i32)
                      n863 = Initialize Array(5.0 ("element"), w608) -> (w604:dbl[])
                      n864 = Initialize Array(5.0 ("element"), w612) -> (w600:dbl[])
                      n865 = call <vilib>:"Cubic Spline Fit.vi"("Y"=w603, "X"=w595, "balance parameter"=-1.0, "Smoothness"=w604) -> ("Best Cubic Spline Fit"=w598:dbl[])  [unwired: 10 in, 1 out]
                      n866 = call <vilib>:"Cubic Spline Fit.vi"("Y"=w599, "X"=w596, "balance parameter"=-1.0, "Smoothness"=w600) -> ("Best Cubic Spline Fit"=w597:dbl[])  [unwired: 10 in, 1 out]
                      n867 = for {
                        tunnel: w598 -> [w618] mode=indexing
                        tunnel: w597 -> [w617] mode=indexing
                        tunnel: w596 -> [w616] mode=indexing
                        tunnel: w595 -> [w615] mode=indexing
                        tunnel: [w614] -> w594 mode=indexing
                        tunnel: [w613] -> w593 mode=indexing
                        n868 = Bundle(w616, "Numeric"=w617) -> (w613:cluster{dbl, "Numeric":dbl})  [unwired: 1 in]
                        n869 = Bundle(w615, "Numeric"=w618) -> (w614:cluster{dbl, "Numeric":dbl})  [unwired: 1 in]
                      }
                      n870 = local write "X calibration"(w594) -> ()
                      n871 = local write "Y calibration"(w593) -> ()
                    }
                    frame True {
                      w627 = cluster{dbl, dbl}[] [{0.0, 0.0}] ("X calibration")
                      n872 = local write "X calibration"(w627) -> ()
                      n873 = local write "Y calibration"(w627) -> ()
                      n874 = local read "ImgData Avg"() -> (w626:T23)
                      n875 = Unbundle By Name(w626) -> ("Centroid Avg"=w625:cluster{"X":sgl, "Y":sgl})
                      n876 = local read "BestRects Cluster"() -> (w629:T12)
                      n877 = Bundle By Name(cluster=w629, "PreviousCenter"=w625, "CurrentCenter"=w625) -> (w628:T12)
                      n878 = local write "BestRects Cluster"(w628) -> ()
                    }
                  }
                }
                event "Add Camera": Mouse Up {
                  n879 = event-data() -> ()  [unwired: 2 out]
                  n880 = local read "DeviceNames"() -> (w630:string[])
                  n881 = call "newCameraPrompt.vi"("DeviceList"=w630) -> ("valid"=w633:bool, "ontrakOut"=w632:i32, "DeviceOut"=w631:string)  [unwired: 8 in]
                  n882 = case shown="True" w633 {
                    tunnel: w632 -> [_ _]
                    tunnel: w631 -> [_ w635]
                    frame False {
                    }
                    frame True {
                      n883 = local read "DeviceNames"() -> (w638:string[])
                      n884 = local write "Add Camera"(FALSE ("Add Camera")) -> ()
                      n885 = local read "AddCameraCluster"() -> (w637:T8)
                      n886 = Search 1D Array(1D array=w638, element=w635) -> (index of element=w639:i32)  [unwired: 1 in]
                      n887 = Bundle By Name(cluster=w637, "Add?"=TRUE, "Device Name"=w635) -> (w634:T8)
                      n888 = local read "Mirrors"() -> (w640:u8[])
                      n889 = Array Size(array=w640) -> (size(s)=w641:i32)
                      n890 = Insert Into Array(array=w640, new element=w639) -> ()  [unwired: 1 in, 1 out]
                      n891 = local write "AddCameraCluster"(w634) -> ()
                      n892 = Increment(x=w641) -> (x+1=w642:i32)
                      n893 = local write "# of cams"(w642) -> ()
                      n894 = property on="Mirrors" class="Arr (strict)"("Number of Rows"=w642) -> ()  [unwired: 2 in, 2 out]
                    }
                  }
                }
                event "Remove Camera": Mouse Up {
                  n895 = event-data() -> ()  [unwired: 2 out]
                  n896 = local read "CamConfigArray"() -> (w645:T9)
                  n897 = local read "Mirrors"() -> (w653:u8[])
                  n898 = property on="USB cameras" class="LstBox (strict)"() -> ("Value"=w646:i32)  [unwired: 2 in, 2 out]
                  n899 = local read "Mirrors"() -> (w655:u8[])
                  n900 = Delete From Array(array=w655, length=1, index=w646) -> (array with subset deleted=w647:u8[])  [unwired: 1 out]
                  n901 = Delete From Array(array=w645, length=1, index=w646) -> (array with subset deleted=w644:T9)  [unwired: 1 out]
                  n902 = Delete From Array(array=w653, length=1, index=w646) -> (array with subset deleted=w652:u8[])  [unwired: 1 out]
                  n903 = local write "Mirrors"(w652) -> ()
                  n904 = local write "CamConfigArray"(w644) -> ()
                  n905 = local write "Mirrors"(w647) -> ()
                  n906 = for {
                    tunnel: [w658] -> w649 mode=indexing
                    tunnel: w647 -> [w657] mode=indexing
                    n907 = local read "DeviceList"() -> (w656:T16)
                    n908 = call "NumberToDeviceID-v2.vi"("device raw"=w657, "DeviceList"=w656) -> ("Name"=w658:string)  [unwired: 5 in, 4 out]
                  }
                  n909 = local write "Remove Camera"(FALSE ("RunON/OFF")) -> ()
                  n910 = property on="USB cameras" class="LstBox (strict)"("Item Names"=w649) -> ()  [unwired: 2 in, 2 out]
                }
                event "USB cameras", "Acquisition Parameters", "Acquisition Parameters dx": Value Change {
                  n911 = event-data() -> ()  [unwired: 7 out]
                  n912 = stacked-sequence {
                    frame #0 {
                      # "stop the main loop"
                      n913 = local write "RunON/OFF"(FALSE ("RunON/OFF")) -> ()
                    }
                    frame #1 {
                      n914 = while {
                        stop <- w660 stop-if-true
                        # "wait until the current camera stop\nto acquire"
                        n915 = Wait (ms)(milliseconds to wait=u32 200) -> ()  [unwired: 1 out]
                        n916 = local read "CloseCam"() -> (w660:bool)
                      }
                    }
                    frame #2 {
                      # "run the main loop with the new camera"
                      n917 = local write "RunON/OFF"(TRUE ("RunON/OFF")) -> ()
                    }
                  }
                }
                event "USB/RS170 cams": Value Change {
                  n918 = event-data() -> ()  [unwired: 7 out]
                  n919 = local write "restart"(TRUE ("Stop")) -> ()
                  n920 = local write "RunON/OFF"(FALSE ("RunON/OFF")) -> ()
                  n921 = local write "stop"(TRUE ("Stop")) -> ()
                }
                event "LoopMode": Value Change {
                  n922 = event-data() -> ("NewVal"=w670:bool)  [unwired: 1 out]
                  n923 = local write "RunON/OFF"(w670) -> ()
                  n924 = Not(x=w670) -> (.not. x?=w671:bool)
                  n925 = local read "# of cams"() -> (w668:i32)
                  n926 = property on="USB cameras Indic" class="LstBox (strict)"("Visible"=w670) -> ()  [unwired: 2 in, 2 out]
                  n927 = call-poly "Replace Or Add.vi"("String"="Acquired Image" ("new element/subarray"), "Index"=w668, "Array In"=w666) -> ()  [unwired: 8 in, 1 out]
                  n928 = property on="Manual Move" class="Clust"("Visible"=w671) -> ()  [unwired: 2 in, 2 out]
                  n929 = local read "Image Selector"() -> (w667:u16)
                  n930 = property on="Image Selector" class="Ring (strict)"("Val(Sgnl)"=w667) -> ()  [unwired: 2 in, 2 out]
                }
                event "Display": Value Change {
                  n931 = event-data() -> ("NewVal"=w677:T26)  [unwired: 1 out]
                  n932 = local read "Display Current"() -> (w673:bool)
                  n933 = Unbundle By Name(w677) -> ("Show Centroid"=w679:bool)
                  n934 = Unbundle By Name(w677) -> ("Show Target Area"=w672:bool)
                  n935 = Unbundle By Name(w677) -> ("Show Target"=w686:bool)
                  n936 = And(x=w679, y=w673) -> (x .and. y?=w680:bool)
                  n937 = property on="Displayed Image" class="IntGraph (strict)"("Active Cursor"=u32 1 ("Active Plot"), "Cursor.Visible"=w686, "Active Cursor"=u32 3 ("Active Plot"), "Cursor.Visible"=w680, "Active Cursor"=u32 4 ("Active Plot"), "Cursor.Visible"=w672, "Active Cursor"=u32 5 ("Active Plot"), "Cursor.Visible"=w672) -> ()  [unwired: 2 in, 2 out]
                  n938 = Unbundle By Name(w677) -> ("Show Avg Centroid"=w675:bool)
                  n939 = Unbundle By Name(w677) -> ("Show Best Rect"=w674:bool)
                  n940 = And(x=w674, y=w673) -> (x .and. y?=w678:bool)
                  n941 = property on="Displayed Image" class="IntGraph (strict)"("Active Cursor"=u32 6 ("Active Plot"), "Cursor.Visible"=w678, "Active Cursor"=u32 7 ("Active Plot"), "Cursor.Visible"=w678, "Active Cursor"=u32 2 ("Active Plot"), "Cursor.Visible"=w675) -> ()  [unwired: 2 in, 2 out]
                }
                event "Fancy Display Options.Use fancy display": Value Change {
                  n942 = event-data() -> ("NewVal"=w688:bool, "OldVal"=w689:bool)  [unwired: 1 out]
                  n943 = property on="Displayed Image" class="IntGraph (strict)"("Visible"=w689) -> ()  [unwired: 2 in, 2 out]
                  n944 = property on="Fancy Display" class="Pict"("Visible"=w688) -> ()  [unwired: 2 in, 2 out]
                }
                event "restart": Value Change {
                  # "if stop set to true, stop the main loop"
                  n945 = event-data() -> ("NewVal"=w691:bool)  [unwired: 6 out]
                  n946 = Not(x=w691) -> (.not. x?=w690:bool)
                  n947 = local write "RunON/OFF"(w690) -> ()
                }
                event "Auto": Value Change {
                  n948 = event-data() -> ()  [unwired: 7 out]
                  n949 = stacked-sequence {
                    frame #0 {
                      n950 = local write "RunON/OFF"(FALSE ("RunON/OFF")) -> ()
                    }
                    frame #1 {
                      n951 = Wait (ms)(milliseconds to wait=u32 100) -> ()  [unwired: 1 out]
                    }
                    frame #2 {
                      n952 = local write "RunON/OFF"(TRUE ("RunON/OFF")) -> ()
                    }
                  }
                }
                event "stop": Value Change {
                  n953 = event-data() -> ()  [unwired: 7 out]
                  n954 = local write "restart"(TRUE ("restart")) -> ()
                  n955 = local write "RunON/OFF"(FALSE ("restart")) -> ()
                }
                event "# imgs to avg": Value Change {
                  n956 = event-data() -> ("OldVal"=w698:i32)  [unwired: 6 out]
                  n957 = local write "# imgs to avg"(w698) -> ()
                  n958 = local write "Status"("Stop and restart to change this value." ("status")) -> ()
                }
                event "Correction Parameters.Movement Type": Value Change {
                  n959 = event-data() -> ("NewVal"=w700:u16)  [unwired: 1 out]
                  n960 = case shown="0, Default" w700 {
                    tunnel: ["Steps" "Scalers"] -> w699
                    frame 0, Default {
                    }
                    frame 1 {
                    }
                  }
                  n961 = property on="X" class="DigNum (strict)"("Caption.Text"=w699) -> ()  [unwired: 2 in, 2 out]
                  n962 = property on="Y" class="DigNum (strict)"("Caption.Text"=w699) -> ()  [unwired: 2 in, 2 out]
                }
                event "Select ROI": Value Change {
                  n963 = event-data() -> ()  [unwired: 2 out]
                  n964 = local read "Acq Img"() -> (w713:T1)
                  n965 = local read "error CamS"() -> (w712:errorcluster)
                  n966 = call "IMAQ Select Rectangle"("error in (no error)"=w712, "Image In"=w713) -> ("error out"=w711:errorcluster, "Cancelled"=w703:bool, "Rectangle"=w710:T13)  [unwired: 6 in, 1 out]
                  n967 = local write "error CamS"(w711) -> ()
                  n968 = Unbundle(w710) -> ("Left"=w709:i32, "Top"=w708:i32, "Right"=w707:i32, "Bottom"=w706:i32)  [unwired: 1 out]
                  n969 = Build Array(w709, w708, w707, w706) -> (w705:i32[])
                  n970 = Select(t=i32[] [0, 0, 0, 0] ("Region of Interest"), s=w703, f=w705) -> (s? t:f=w714:i32[])
                  n971 = property on="Region of Interest" class="Arr (strict)"("Val(Sgnl)"=w714) -> ()  [unwired: 2 in, 2 out]
                  n972 = local write "Select ROI"(FALSE ("Select ROI")) -> ()
                }
                event "Reset ROI": Value Change {
                  n973 = event-data() -> ()  [unwired: 2 out]
                  n974 = Initialize Array(0 ("element"), 4 ("dimension size")) -> (w719:i32[])
                  n975 = local write "Region of Interest"(w719) -> ()
                  n976 = local write "Reset ROI"(FALSE ("Reset ROI")) -> ()
                }
                event "Image Selector": Value Change {
                  n977 = event-data() -> ("NewVal"=w725:u16)  [unwired: 1 out]
                  n978 = local read "LoopMode"() -> (w724:bool)
                  n979 = local read "# of cams"() -> (w726:i32)
                  n980 = Not Equal?(x=w725, y=w726) -> (x != y?=w723:bool)
                  n981 = And(x=w723, y=w724) -> (x .and. y?=w722:bool)
                  n982 = Not(x=w722) -> (.not. x?=w721:bool)
                  n983 = local write "Display Current"(w721) -> ()
                  n984 = local read "Display"() -> (w720:T26)
                  n985 = property on="Display" class="Clust (strict)"("Val(Sgnl)"=w720) -> ()  [unwired: 2 in, 2 out]
                }
                event "Auto Detect Param": Value Change {
                  n986 = event-data() -> ("NewVal"=w732:bool)  [unwired: 6 out]
                  n987 = local read "Select ROI"() -> (w730:bool)
                  n988 = Not(x=w730) -> (.not. x?=w728:bool)
                  n989 = Not(x="LoopMode") -> (.not. x?=w729:bool)
                  n990 = Compound Arithmetic op=AND(w732, w729, w728) -> (w731:bool)
                  n991 = case shown="False" w731 {
                    selector: w731 -> [w733 _]
                    frame False {
                      n992 = local write "Auto Detect Param"(w733) -> ()
                      n993 = local write "Status"("Auto Detect Param\n unable in automatic mode\nor when select ROI is on." ("status")) -> ()
                    }
                    frame True {
                      n994 = local write "RunON/OFF"(TRUE ("Substract Background")) -> ()
                    }
                  }
                }
                event "Grab Backround Image": Mouse Up {
                  w747 = FALSE ("Visible")
                  n995 = event-data() -> ()  [unwired: 9 out]
                  n996 = property on="Image to save" class="IntGraph (strict)"("Visible"=TRUE) -> ()  [unwired: 2 in, 2 out]
                  n997 = property on="Grab reference Image" class="Bool (strict)"("Visible"=w747) -> ()  [unwired: 2 in, 2 out]
                  n998 = property on="Grab Backround Image" class="Bool (strict)"("Visible"=w747) -> ()  [unwired: 2 in, 2 out]
                  n999 = property on="Base Directory" class="Path"("Visible"=w747) -> ()  [unwired: 2 in, 2 out]
                  n1000 = property on="SavePict" class="Bool (strict)"("Visible"=w747) -> ()  [unwired: 2 in, 2 out]
                  n1001 = local read "Acq Img"() -> (w739:T1)
                  n1002 = local read "CamConfigArray"() -> (w742:T9)
                  n1003 = local read "USB cameras"() -> (w741:i32)
                  n1004 = local read "Buffer"() -> (w740:T1)
                  n1005 = call "IMAQ ImageToArray"("Image"=w739) -> ("Image Pixels (U8)"=w744:u8[][])  [unwired: 3 in, 4 out]
                  n1006 = call "IMAQ Copy"("Image Dst"=w740, "Image Src"=w739) -> ()  [unwired: 4 in, 2 out]
                  n1007 = local write "Image to save"(w744) -> ()
                  n1008 = call "Display Message Background"() -> ("OK"=w746:bool)  [unwired: 10 in, 1 out]
                  n1009 = Index Array(array=w742, index=w741) -> (element=w743:T36)
                  n1010 = case shown="False" w746 {
                    tunnel: [TRUE ("Visible") TRUE ("Visible")] -> w745
                    tunnel: w743 -> [_ w752]
                    frame False {
                    }
                    frame True {
                      n1011 = local read "Buffer"() -> (w751:T1)
                      n1012 = local read "Background Img"() -> (w753:T1)
                      n1013 = call "Save Background Img.vi"("Acq Img"=w751, "CamConfigCluster"=w752) -> ("Background Path"=w749:path)  [unwired: 9 in]
                      n1014 = call "IMAQ Copy"("Image Dst"=w753, "Image Src"=w751) -> ("Image Dst Out"=w750:T1)  [unwired: 4 in, 1 out]
                      n1015 = local write "Background Path"(w749) -> ()
                      n1016 = local write "Background Img"(w750) -> ()
                    }
                  }
                  n1017 = local write "Grab Backround Image"(FALSE ("Grab Backround Image")) -> ()
                  n1018 = Not(x=w745) -> (.not. x?=w736:bool)
                  n1019 = property on="Grab reference Image" class="Bool (strict)"("Visible"=w745) -> ()  [unwired: 2 in, 2 out]
                  n1020 = property on="Grab Backround Image" class="Bool (strict)"("Visible"=w745) -> ()  [unwired: 2 in, 2 out]
                  n1021 = property on="Base Directory" class="Path"("Visible"=w745) -> ()  [unwired: 2 in, 2 out]
                  n1022 = property on="SavePict" class="Bool (strict)"("Visible"=w745) -> ()  [unwired: 2 in, 2 out]
                  n1023 = property on="Image to save" class="IntGraph (strict)"("Visible"=w736) -> ()  [unwired: 2 in, 2 out]
                }
                event "Grab reference Image": Mouse Up {
                  w767 = FALSE ("Visible")
                  n1024 = event-data() -> ()  [unwired: 9 out]
                  n1025 = property on="Image to save" class="IntGraph (strict)"("Visible"=TRUE) -> ()  [unwired: 2 in, 2 out]
                  n1026 = property on="Grab reference Image" class="Bool (strict)"("Visible"=w767) -> ()  [unwired: 2 in, 2 out]
                  n1027 = property on="Grab Backround Image" class="Bool (strict)"("Visible"=w767) -> ()  [unwired: 2 in, 2 out]
                  n1028 = property on="Base Directory" class="Path"("Visible"=w767) -> ()  [unwired: 2 in, 2 out]
                  n1029 = property on="SavePict" class="Bool (strict)"("Visible"=w767) -> ()  [unwired: 2 in, 2 out]
                  n1030 = local read "CamConfigArray"() -> (w761:T9)
                  n1031 = local read "Acq Img"() -> (w760:T1)
                  n1032 = local read "USB cameras"() -> (w762:i32)
                  n1033 = local read "Buffer"() -> (w759:T1)
                  n1034 = call "IMAQ ImageToArray"("Image"=w760) -> ("Image Pixels (U8)"=w764:u8[][])  [unwired: 3 in, 4 out]
                  n1035 = local write "Image to save"(w764) -> ()
                  n1036 = call "IMAQ Copy"("Image Dst"=w759, "Image Src"=w760) -> ("Image Dst Out"=w755:T1)  [unwired: 4 in, 1 out]
                  n1037 = local write "Buffer"(w755) -> ()
                  n1038 = Index Array(array=w761, index=w762) -> (element=w763:T36)
                  n1039 = call "Display Message Reference"() -> ("OK"=w766:bool)  [unwired: 10 in, 1 out]
                  n1040 = case shown="False" w766 {
                    tunnel: [TRUE ("Visible") TRUE ("Visible")] -> w765
                    tunnel: w763 -> [_ w770]
                    frame False {
                    }
                    frame True {
                      n1041 = local read "Buffer"() -> (w771:T1)
                      n1042 = local read "Reference Img"() -> (w773:T1)
                      n1043 = call "Save Reference Img.vi"("Acq Img"=w771, "CamConfigCluster"=w770) -> ("Reference Path"=w772:path)  [unwired: 9 in]
                      n1044 = local write "Reference Path"(w772) -> ()
                      n1045 = call "IMAQ Copy"("Image Dst"=w773, "Image Src"=w771) -> ("Image Dst Out"=w769:T1)  [unwired: 4 in, 1 out]
                      n1046 = local write "Reference Img"(w769) -> ()
                    }
                  }
                  n1047 = local write "Grab reference Image"(FALSE ("Grab reference Image")) -> ()
                  n1048 = Not(x=w765) -> (.not. x?=w756:bool)
                  n1049 = property on="Grab reference Image" class="Bool (strict)"("Visible"=w765) -> ()  [unwired: 2 in, 2 out]
                  n1050 = property on="Grab Backround Image" class="Bool (strict)"("Visible"=w765) -> ()  [unwired: 2 in, 2 out]
                  n1051 = property on="Base Directory" class="Path"("Visible"=w765) -> ()  [unwired: 2 in, 2 out]
                  n1052 = property on="SavePict" class="Bool (strict)"("Visible"=w765) -> ()  [unwired: 2 in, 2 out]
                  n1053 = property on="Image to save" class="IntGraph (strict)"("Visible"=w756) -> ()  [unwired: 2 in, 2 out]
                }
                event "Set Color Map": Value Change {
                  n1054 = event-data() -> ("NewVal"=w775:bool)  [unwired: 1 out]
                  n1055 = case shown="True" w775 {
                    frame False {
                    }
                    frame True {
                      n1056 = call "Color Table Generator.vi"() -> ("Color Map"=w776:u32[])
                      n1057 = property on="Displayed Image" class="IntGraph (strict)"("Color Table"=w776) -> ()  [unwired: 2 in, 2 out]
                    }
                  }
                }
                event "Open CamCenter": Value Change {
                  n1058 = event-data() -> ("NewVal"=w777:bool)  [unwired: 1 out]
                  n1059 = case shown="True" w777 {
                    frame False {
                    }
                    frame True {
                      # "open creative live! cam center"
                      n1060 = call <vilib>:"System Exec.vi"("wait until completion? (T)"=FALSE, "command line"="open \"C:\\BeamPointing\\trunk\\Beam Poin\nting v22 Library\\xml Settings\\ConfigFile.xml\"") -> ("error out"=w778:errorcluster)  [unwired: 4 in, 5 out]
                      n1061 = call <vilib>:"Simple Error Handler.vi"("error in (no error)"=w778) -> ()  [unwired: 4 in, 5 out]
                    }
                  }
                }
              }
            }
            n1062 = case shown="False" "newMC" {
              tunnel: [w433 w444] -> w428
              tunnel: [w432 w443] -> w426
              tunnel: w424 -> [w431 w441]
              frame True {
                n1063 = for {
                  tunnel: "image::" ("image prefix") -> [w438]
                  tunnel: w431 -> [_] mode=indexing
                  tunnel: [w439] -> w433 mode=indexing
                  tunnel: [w437] -> w432 mode=indexing
                  i -> [w436]
                  n1064 = Increment(x=w436) -> (x+1=w435:i32)
                  n1065 = Number To Decimal String(number=w435) -> (decimal integer string=w434:string)  [unwired: 1 in]
                  n1066 = Concatenate Strings(w438, w434) -> (w437:string)
                  n1067 = Type Cast(type=T1 refnum ("New Image"), x=w437) -> (*(type *) &x=w439:T1)
                }
              }
              frame False {
                n1068 = for {
                  tunnel: "image prefix 2" -> [w446]
                  tunnel: w441 -> [w448] mode=indexing
                  tunnel: [w447] -> w444 mode=indexing
                  tunnel: [w445] -> w443 mode=indexing
                  n1069 = Number To Decimal String(number=w448) -> (decimal integer string=w449:string)  [unwired: 1 in]
                  n1070 = Concatenate Strings(w446, w449) -> (w445:string)
                  n1071 = Type Cast(type=T1 refnum ("New Image"), x=w445) -> (*(type *) &x=w447:T1)
                }
              }
            }
            "image names" <- w426
            n1072 = while {
              tunnel: w428 -> [w460]
              tunnel: w425 -> [w453]
              tunnel: w424 -> [w452]
              tunnel: "newMC" -> [w451]
              i -> [w455]
              stop <- w458 stop-if-true
              n1073 = Equal To 0?(x=w455) -> (x = 0?=w456:bool)
              n1074 = Or(x="Stop 2", y=w456) -> (x .or. y?=w454:bool)
              n1075 = case shown="True" w451 {
                tunnel: w454 -> [w497 _]
                tunnel: w453 -> [w496 _]
                tunnel: w452 -> [w495 _]
                frame False {
                  n1076 = case shown="True" w497 {
                    tunnel: w496 -> [_ w499]
                    tunnel: w495 -> [_ w498]
                    frame False {
                    }
                    frame True {
                      n1077 = stacked-sequence {
                        tunnel: w499 -> [_ w503]
                        tunnel: w498 -> [_ w502]
                        frame #0 {
                          n1078 = local read "TCP IDs"() -> (w501:refnum<k5>[])
                          n1079 = local write "Stop 2"(FALSE ("Stop 2")) -> ()
                          n1080 = call "TCP multi close.vi"("TCP Ports"=w501) -> ()
                        }
                        frame #1 {
                          n1081 = Number To Decimal String(number=w502) -> (decimal integer string=w506:string[])  [unwired: 1 in]
                          n1082 = call "TCP multiple open.vi"("timeout ms (60000)"=2000, "Ports"=w506, "IP Addresses"=w503) -> ("Array"=→"TCP IDs":refnum<k5>[])  [unwired: 1 in, 1 out]
                        }
                      }
                    }
                  }
                }
                frame True {
                }
              }
              n1083 = local read "Image client connect errors"() -> (w479:errorcluster[])
              n1084 = local read "USB cameras"() -> (w476:i32)
              n1085 = local read "Raw images"() -> (w493:T1[])
              n1086 = local read "CamConfigArray"() -> (w480:T9)
              n1087 = call "Select Target Circle Colors.vi"("USB cameras"=w476, "Image client connect errors"=w479) -> ("Array"=w478:u32[])
              n1088 = local read "UDP connect array"() -> (w491:refnum<k16>[])
              n1089 = local read "Ann. Images"() -> (w472:T1[])
              n1090 = local read "Detection status"() -> (w474:string[])
              n1091 = Array Size(array=w493) -> (size(s)=w492:i32)
              n1092 = for {
                workers-P: w492 -> [_]
                tunnel: w493 -> [w542] mode=indexing
                tunnel: w491 -> [w541] mode=indexing
                tunnel: [w539] -> w471 mode=indexing
                tunnel: [w536] -> w481 mode=indexing
                tunnel: w479 -> [w540] mode=indexing
                tunnel: w480 -> [w538] mode=indexing
                tunnel: [w535] -> w470 mode=indexing
                tunnel: w478 -> [w534] mode=indexing
                tunnel: "CamOn" -> [w533] mode=indexing
                tunnel: w474 -> [w532] mode=indexing
                tunnel: "UDP timeout ms" -> [w531]
                tunnel: w472 -> [w530] mode=indexing
                tunnel: w460 -> [w529] mode=indexing
                tunnel: bool[] [FALSE, FALSE, FALSE, FALSE, FALSE, FALSE, FALSE, FALSE, FALSE] -> [w528] mode=indexing
                i -> [w537]
                n1093 = case shown="True" w533 {
                  tunnel: w542 -> [_ w559]
                  tunnel: w541 -> [_ w558]
                  tunnel: w540 -> [w544 _]
                  tunnel: [w543 w554] -> w539
                  tunnel: w538 -> [_ w557]
                  tunnel: [w544 w556] -> w536
                  tunnel: [_ w551] -> w535
                  tunnel: w534 -> [_ w553]
                  tunnel: w532 -> [_ w552]
                  tunnel: w531 -> [_ w550]
                  tunnel: w530 -> [w543 w549]
                  tunnel: w529 -> [_ w547]
                  tunnel: w528 -> [_ w545]
                  frame False {
                  }
                  frame True {
                    n1094 = case shown="No Error" errorcluster {"status"=FALSE, "code"=0, "source"=""} ("error IO") {
                      selector: errorcluster {"status"=FALSE, "code"=0, "source"=""} ("error IO") -> [_ w578]
                      tunnel: w559 -> [w567 w579]
                      tunnel: w558 -> [w566 _]
                      tunnel: [w565 w578] -> w556
                      tunnel: [w564 w579] -> w555
                      tunnel: [w563 FALSE ("status")] -> w551
                      tunnel: w550 -> [w562 _]
                      tunnel: w547 -> [w561 _]
                      tunnel: w545 -> [w560 _]
                      frame No Error {
                        n1095 = case shown="True" w560 {
                          tunnel: w567 -> [w568 w576]
                          tunnel: w566 -> [_ w575]
                          tunnel: [_ w574] -> w565
                          tunnel: [w570 w573] -> w564
                          tunnel: [_ w572] -> w563
                          tunnel: w562 -> [_ w571]
                          tunnel: w561 -> [w569 _]
                          frame False {
                            n1096 = call "IMAQ Copy"("Image Dst"=w568, "Image Src"=w569) -> ("Image Dst Out"=w570:T1)  [unwired: 4 in, 1 out]
                          }
                          frame True {
                            n1097 = call "GrabImageUDP.vi"("Image in"=w576, "connection ID"=w575, "timeout ms (25000)"=w571) -> ("Image Out"=w573:T1, "error out"=w574:errorcluster, "status"=w572:bool)  [unwired: 10 in]
                          }
                        }
                      }
                      frame Error {
                      }
                    }
                    n1098 = call "annotate image.vi"("Detection string"=w552, "Color"=w553, "CamConfigArray"=w557, "rescale"="rescale", "Image Dst"=w549, "Image in"=w555) -> ("Image Dst Out"=w554:T1)  [unwired: 4 in, 1 out]
                  }
                }
                "grab loop i" <- w537
              }
              "Image client grab errors" <- w481
              "Timeout" <- w470
              n1099 = local write "Ann. Images"(w471) -> ()
              n1100 = Index Array(array=w470) -> (element #1=→"1":bool, element #2=→"1 2":bool, element #3=→"1 3":bool, element #4=→"1 4":bool, element #5=→"1 5":bool, element #6=→"1 6":bool, element #7=→"1 7":bool, element #8=→"1 8":bool, element #9=→"1 9":bool)  [unwired: 9 in]
              n1101 = Index Array(array=w471) -> (element #1=→"Image":T1, element #2=→"Image 2":T1, element #3=→"Image 3":T1, element #4=→"Image 4":T1, element #5=→"Image 5":T1, element #6=→"Image 6":T1, element #7=→"Image 7":T1, element #8=→"Image 8":T1, element #9=→"Image 9":T1)  [unwired: 9 in]
              n1102 = Wait (ms)(milliseconds to wait=u32 100) -> ()  [unwired: 1 out]
              n1103 = case shown="False" "recenter" {
                frame False {
                }
                frame True {
                  n1104 = control-ref of="Image"() -> (w510:refnum<vi>)
                  n1105 = control-ref of="Image 2"() -> (w512:refnum<vi>)
                  n1106 = control-ref of="Image 3"() -> (w513:refnum<vi>)
                  n1107 = control-ref of="Image 4"() -> (w514:refnum<vi>)
                  n1108 = control-ref of="Image 5"() -> (w515:refnum<vi>)
                  n1109 = control-ref of="Image 6"() -> (w516:refnum<vi>)
                  n1110 = control-ref of="Image 7"() -> (w517:refnum<vi>)
                  n1111 = control-ref of="Image 8"() -> (w518:refnum<vi>)
                  n1112 = control-ref of="Image 9"() -> (w519:refnum<vi>)
                  n1113 = local read "CamConfigArray"() -> (w508:T9)
                  n1114 = local write "recenter"(FALSE ("recenter")) -> ()
                  n1115 = Build Array(w510, w512, w513, w514, w515, w516, w517, w518, w519) -> (w511:refnum<vi>[])
                  n1116 = for {
                    tunnel: w511 -> [w527] mode=indexing
                    tunnel: w508 -> [w526] mode=indexing
                    n1117 = Unbundle By Name(w526) -> ("CorrectConfig Cluster.Target"=w525:cluster{"X Target":sgl, "Y Target":sgl}, "CorrectConfig Cluster.Detection Parameters.Rx"=w522:i32)
                    n1118 = Reciprocal(x=w522) -> (1/x=w521:dbl)
                    n1119 = Divide(x=w521, y=0.01 ("1/x")) -> (x/y=w523:dbl)
                    n1120 = Bundle(w523, w523) -> (w524:cluster{dbl, dbl})  [unwired: 1 in]
                    n1121 = property class="ImageControl"(reference=w527, "ZoomSingle"=w524, "Image Center Position"=w525) -> ()  [unwired: 1 in, 2 out]
                  }
                }
              }
              n1122 = local read "restart"() -> (w458:bool)
              n1123 = case shown="False" w458 {
                frame False {
                }
                frame True {
                  n1124 = local read "TCP IDs"() -> (w507:refnum<k5>[])
                  n1125 = call "TCP multi close.vi"("TCP Ports"=w507) -> ()
                }
              }
            }
            n1126 = while {
              stop <- w783 stop-if-true
              # "TCP reception from picodrivers server"
              n1127 = local read "ConnectArray"() -> (w784:T7)
              n1128 = local read "restart"() -> (w783:bool)
              n1129 = for {
                tunnel: w784 -> [w793] mode=indexing
                i -> [w786]
                n1130 = Unbundle(w793) -> ("connection ID"=w792:refnum<k5>, "TCP error"=w789:errorcluster)  [unwired: 2 out]
                n1131 = Wait (ms)(milliseconds to wait=u32 200) -> ()  [unwired: 1 out]
                n1132 = call "TCPread8bytes.vi"("Error in"=w789, "timeout ms (25000)"=500, "connection ID in"=w792) -> ("Error out"=w787:errorcluster, "string out"=w790:string, "connection ID out"=w785:refnum<k5>)  [unwired: 6 out]
                n1133 = case shown="\"close\"" w790 {
                  selector: w790 -> [w794 _ w804]
                  tunnel: w787 -> [w797 _ w808]
                  tunnel: w786 -> [w799 _ _]
                  tunnel: w785 -> [_ _ w809]
                  frame Default {
                    n1134 = local write "Status"(w794) -> ()
                    n1135 = local read "InProgress"() -> (w796:string[])
                    n1136 = Decrement(x=w799) -> (x-1=w798:i32)
                    n1137 = Unbundle By Name(w797) -> ("status"=w802:bool)
                    n1138 = local read "ConnectArray"() -> (w800:T7)
                    n1139 = Not(x=w802) -> (.not. x?=w803:bool)
                    n1140 = call "EndOfMove-2.vi"("InProgressIN"=w796, "String in"=w794) -> ("InProgressOUT"=w795:string[])  [unwired: 8 out]
                    n1141 = local write "TCPconnecAnswer"(w803) -> ()
                    n1142 = local write "InProgress"(w795) -> ()
                    n1143 = call "LoadConnectionIDerror.vi"("ArrayIN"=w800, "ErrorIn"=w797, "index"=w798) -> ("ArrayOUT"=w801:T7)  [unwired: 8 out]
                    n1144 = local write "ConnectArray"(w801) -> ()
                  }
                  frame "" {
                  }
                  frame "close" {
                    n1145 = local write "Status"(w804) -> ()
                    n1146 = TCP Close Connection(connection ID=w809, error in (no error)=w808) -> (connection ID out=w807:refnum<k5>)  [unwired: 2 out]
                    n1147 = local read "ConnectArray"() -> (w806:T7)
                    n1148 = call "RemoveConnectionID.vi"("ArrayIN"=w806, "connection ID"=w807) -> ("ArrayOUT"=w805:T7)  [unwired: 9 out]
                    n1149 = local write "ConnectArray"(w805) -> ()
                  }
                }
              }
              n1150 = local read "InProgress"() -> (w782:string[])
              n1151 = call "EndOfMove-2.vi"("InProgressIN"=w782) -> ("InProgress"=w781:bool)  [unwired: 1 in, 8 out]
              n1152 = property on="MoveInProgress" class="Bool (strict)"("Val(Sgnl)"=w781) -> ()  [unwired: 2 in, 2 out]
            }
          }
          frame #2 {
            n1153 = local read "ConnectArray"() -> (w1834:T7)
            n1154 = local write "restart"(FALSE ("stop")) -> ()
            n1155 = for {
              tunnel: w1834 -> [w1886] mode=indexing
              # "close all connection"
              n1156 = Unbundle(w1886) -> ("connection ID"=w1884:refnum<k5>, "TCP error"=w1883:errorcluster)  [unwired: 2 out]
              n1157 = call "TCPwrite8bytes.vi"("Error in"=w1883, "Cmd In"="webcam:close", "connection ID in"=w1884) -> ("Error out"=w1882:errorcluster, "connection ID out"=w1881:refnum<k5>)  [unwired: 7 in]
              n1158 = TCP Close Connection(connection ID=w1881, error in (no error)=w1882) -> (error out=w1885:errorcluster)  [unwired: 2 out]
              n1159 = local write "error close connect"(w1885) -> ()
            }
            n1160 = stacked-sequence {
              frame #0 {
                n1161 = local read "AddCameraCluster"() -> (w1839:T8)
                n1162 = Unbundle By Name(w1839) -> ("Add?"=w1838:bool, "Channel"=w1836:i32, "Device Name"=w1837:string)
                n1163 = case shown="True" w1838 {
                  tunnel: w1837 -> [_ w1840]
                  tunnel: w1836 -> [_ _]
                  frame False {
                  }
                  frame True {
                    w1841 = T36 {"ID"=0.0, "Name"="no-device", "DeviceID"={"Slot Connector"=0, "IP Adress"="Ipaddress", "Port"=0, "Type"="Type"}, "CorrectConfig Cluster"={"Detection Parameters"={"Contrast"=0, "Treshold"=0, "Max Intensity"=0, "Max Intensity%"=0, "Rx"=0, "Ry"=0, "R%"=0.0}, "Reverse"={"Reverse X"=FALSE, "Reverse Y"=FALSE}, "Target"={"X Target"=0.0, "Y Target"=0.0}, "Region of Interest"=[0, 0, 0, 0], "Correction Parameters"={"X"=0.0, "Y"=0.0, "Movement Type"=0}, "Acquisition Parameters"={"Brightness"=0.0, "Contrast"=0.0, "Saturation"=0.0, "White level"=0.0}, "Background Path"=path "", "Reference Path"=path "", "XCalibration"=[], "YCalibration"=[]}, "Ontrak Channel"=0, "IMAQdx Session 2"="cam2", "ImageServer"={"IPAddress"="", "Port"=0}}
                    n1164 = local read "AddCameraCluster"() -> (w1843:T8)
                    n1165 = Bundle By Name(cluster=w1843, "Add?"=FALSE) -> (w1844:T8)
                    n1166 = local write "AddCameraCluster"(w1844) -> ()
                    n1167 = local read "CamConfigArray"() -> (w1846:T9)
                    n1168 = Bundle By Name(cluster=w1841, "Name"=w1840) -> ()  [unwired: 1 out]
                    n1169 = Build Array (concatenate)(w1846, w1841) -> (w1845:T9)
                    n1170 = local write "CamConfigArray"(w1845) -> ()
                  }
                }
              }
              frame #1 {
                n1171 = local read "XML errors"() -> (w1847:bool)
                n1172 = case shown="False" w1847 {
                  frame False {
                    n1173 = stacked-sequence {
                      frame #0 {
                        n1174 = local read "USB/RS170 cams"() -> (w1856:bool)
                        n1175 = local read "Mirror List Path"() -> (w1855:path)
                        n1176 = call "LoadDeviceList.vi"("usb/RS170"=w1856, "path to XML document"=w1855) -> ("DeviceList"=w1857:T16)  [unwired: 7 in, 2 out]
                        n1177 = local read "CamConfigArray"() -> (w1848:T9)
                        n1178 = call "parse device list by type.vi"("DeviceListin"=w1857) -> ("DeviceListout"=w1854:T16)  [unwired: 1 in]
                        n1179 = local read "Mirrors"() -> (w1853:u8[])
                        n1180 = call "associate mirrors and cameras.vi"("Mirrors"=w1853, "DeviceList"=w1854) -> ("CamConfigArray"=w1850:T9)  [unwired: 1 in]
                        n1181 = Not Equal?(x=w1850, y=w1848) -> (x != y?=w1852:bool)
                        "configarraychanged" <- w1852
                        n1182 = case shown="True" w1852 {
                          tunnel: [TRUE ("T button?") w1860] -> w1851
                          frame False {
                          }
                          frame True {
                            n1183 = Two Button Dialog(message="READ! config has changed.\nplease ensure all other BP\ninstances SHARING same\n cameras are shutdown\nbefore saving config.", 1:"Dont save config" ("F button name (\"Cancel\")"), 2:"save" ("T button name (\"OK\")")) -> (T button?=w1860:bool)
                          }
                        }
                        "really save cfg?" <- w1851
                        n1184 = Select(t=w1848, s=w1851, f=w1850) -> (s? t:f=w1849:T9)
                        n1185 = local write "CamConfigArray"(w1849) -> ()
                      }
                      frame #1 {
                        n1186 = local read "really save cfg?"() -> (w1863:bool)
                        n1187 = case shown="True" w1863 {
                          frame False {
                          }
                          frame True {
                            n1188 = local read "CamConfigArray"() -> (w1869:T9)
                            n1189 = local read "Cameras Names"() -> (w1864:string[])
                            n1190 = Array Size(array=w1869) -> (size(s)=w1867:i32)
                            n1191 = Array Size(array=w1864) -> (size(s)=w1866:i32)
                            n1192 = Subtract(x=w1867, y=w1866) -> (x-y=w1868:i32)
                            n1193 = for {
                              N: w1868 -> [_]
                              shift-right: [w1875] -> w1865
                              shift-left: w1864 -> [w1876]
                              n1194 = Build Array (concatenate)(w1876, "Null") -> (w1875:string[])
                            }
                            n1195 = local read "Mirror List Path"() -> (w1874:path)
                            n1196 = local read "XML Config File Path"() -> (w1872:path)
                            n1197 = local read "USB/RS170 cams"() -> (w1873:bool)
                            n1198 = call "SaveCamConfig-v5.vi"("file path in"=w1874, "CamConfigArray"=w1869) -> ("parse errors"=w1870:string)  [unwired: 7 in]
                            n1199 = call "SaveConfig.vi"("path to XML document"=w1872, "USB/RS170 cams"=w1873, "CamerasNames"=w1865, "DeviceConfigArray"=w1869) -> ("error out"=w1871:errorcluster)  [unwired: 7 in]
                            n1200 = local write "Status"(w1870) -> ()
                            n1201 = call <vilib>:"Simple Error Handler.vi"("error in (no error)"=w1871) -> ()  [unwired: 4 in, 5 out]
                          }
                        }
                      }
                    }
                  }
                  frame True {
                  }
                }
              }
              frame #2 {
                n1202 = disable-structure shown="Enabled" {
                  frame Disabled {
                    n1203 = local read "Mirror List Path"() -> (w1879:path)
                    n1204 = local read "XML Config File Path"() -> (w1878:path)
                    n1205 = call "StripEmtyLines.vi"("Path"=w1879) -> ()
                    n1206 = call "StripEmtyLines.vi"("Path"=w1878) -> ()
                  }
                  frame Enabled {
                  }
                }
              }
            }
            n1207 = local read "error CamS"() -> (w1827:errorcluster)
            n1208 = local read "Acq Img"() -> (w1832:T1)
            n1209 = local read "Background Img"() -> (w1823:T1)
            n1210 = local read "Thresh Img"() -> (w1833:T1)
            n1211 = local read "Thresh Img"() -> (w1822:T1)
            n1212 = local read "Thresh Img"() -> (w1820:T1)
            n1213 = local read "Avg Img"() -> (w1831:T1)
            n1214 = call "IMAQ Dispose"("Image"=w1832, "error in (no error)"=w1827) -> ("error out"=w1829:errorcluster)  [unwired: 1 in, 3 out]
            n1215 = call "IMAQ Dispose"("Image"=w1831, "error in (no error)"=w1829) -> ("error out"=w1828:errorcluster)  [unwired: 1 in, 3 out]
            n1216 = call "IMAQ Dispose"("Image"=w1833, "error in (no error)"=w1828) -> ("error out"=w1821:errorcluster)  [unwired: 1 in, 3 out]
            n1217 = call "IMAQ Dispose"("Image"=w1823, "error in (no error)"=w1821) -> ("error out"=w1824:errorcluster)  [unwired: 1 in, 3 out]
            n1218 = call "IMAQ Dispose"("Image"=w1822, "error in (no error)"=w1824) -> ("error out"=w1819:errorcluster)  [unwired: 1 in, 3 out]
            n1219 = call "IMAQ Dispose"("Image"=w1820, "error in (no error)"=w1819) -> ("error out"=w1818:errorcluster)  [unwired: 1 in, 3 out]
            n1220 = local read "UDP connect array"() -> (w1817:refnum<k16>[])
            n1221 = for {
              tunnel: w1817 -> [w1835] mode=indexing
              n1222 = UDP Close(connection ID=w1835) -> ()  [unwired: 1 in, 2 out]
            }
            n1223 = call <vilib>:"Clear Errors.vi"("error in (no error)"=w1818) -> ("error out"=w1826:errorcluster)  [unwired: 6 in]
            n1224 = local write "error CamS"(w1826) -> ()
            n1225 = local read "stop"() -> (w1825:bool)
          }
        }
      }
    }
    frame #2 {
      n1226 = local read "Raw images"() -> (w1889:T1[])
      n1227 = local read "XML Config File Path"() -> (w1888:path)
      n1228 = local read "Mirror List Path"() -> (w1887:path)
      n1229 = for {
        tunnel: w1889 -> [w1891] mode=indexing
        n1230 = call "IMAQ Dispose"("Image"=w1891) -> ()  [unwired: 2 in, 4 out]
      }
      n1231 = local write "stop"(FALSE ("Stop")) -> ()
      n1232 = call "StripEmtyLines.vi"("Path"=w1887) -> ()
      n1233 = call "StripEmtyLines.vi"("Path"=w1888) -> ()
    }
  }
  n1234 = local read "newMC"() -> (w9:bool)
  n1235 = case shown="False" w9 {
    frame False {
      n1236 = while {
        stop <- w1892 stop-if-true
        # "Check for errors minus the connection closed error."
        # "Notify the server that we are stopping by passing a byte back to the Read the date and time data being sent by the Date & Time Server.vi then close connection."
        # "Read the date and time data being sent by the Date & Time Server.vi.  First TCP Read gathers bytes to read and passes it to the second TCP read which outputs the date & time string."
        # "Open Connection with Port number and Machine name."
        n1237 = local read "image names"() -> (w1893:string[])
        n1238 = local read "TCP IDs"() -> (w1896:refnum<k5>[])
        n1239 = Array Size(array=w1896) -> (size(s)=w1894:i32)
        n1240 = Not Equal To 0?(x=w1894) -> (x != 0?=w1895:bool)
        n1241 = case shown="True" w1895 {
          tunnel: w1896 -> [_ w1899]
          tunnel: w1894 -> [_ w1898]
          tunnel: w1893 -> [_ w1897]
          frame False {
          }
          frame True {
            n1242 = for {
              tunnel: w1899 -> [w1907] mode=indexing
              workers-P: w1898 -> [_]
              tunnel: w1897 -> [w1902] mode=indexing
              w1904 = T35 0 items=["Grayscale (U8)", "Grayscale (I16)", "Grayscale (SGL)", "Complex (CSG)", "RGB (U32)", "HSL (U32)", "RGB (U64)", "Grayscale (U16)"] ("Image Type")
              w1910 = T35 0 items=["Grayscale (U8)", "Grayscale (I16)", "Grayscale (SGL)", "Complex (CSG)", "RGB (U32)", "HSL (U32)", "RGB (U64)", "Grayscale (U16)"] ("Image Type")
              n1243 = Concatenate Strings(w1902, "tmp" ("string")) -> (w1900:string)
              n1244 = call "IMAQ Create"("Image Name"=w1900, "Image Type"=w1904) -> ("New Image"=w1903:T1)  [unwired: 3 in, 1 out]
              n1245 = call "IMAQ Create"("Image Name"=w1902, "Image Type"=w1910) -> ("New Image"=w1909:T1)  [unwired: 3 in, 1 out]
              n1246 = while {
                tunnel: [w1937] -> _
                tunnel: [w1918] -> _
                tunnel: w1907 -> [w1912]
                shift-right: [w1927] -> w1906
                shift-left: w1909 -> [w1928]
                shift-right: [w1926] -> w1905
                shift-left: w1903 -> [w1925]
                tunnel: -1 ("timeout ms (25000)") -> [w1919]
                stop <- w1936 stop-if-true
                w1934 = 4
                n1247 = TCP Read(connection ID=w1912, bytes to read=w1934, 9:w1919) -> (connection ID out=w1930:refnum<k5>, data out=w1933:string, error out=w1931:errorcluster)  [unwired: 2 in]
                n1248 = Type Cast(type=w1934, x=w1933) -> (*(type *) &x=w1932:i32)
                n1249 = Wait (ms)(milliseconds to wait=u32 50) -> ()  [unwired: 1 out]
                n1250 = TCP Read(connection ID=w1930, bytes to read=w1932, error in (no error)=w1931, 9:w1919) -> (connection ID out=w1937:refnum<k5>, data out=w1929:string, error out=w1921:errorcluster)  [unwired: 1 out]
                n1251 = Unbundle By Name(w1921) -> ("code"=w1924:i32)
                n1252 = Equal?(x=w1924, y=56) -> (x = y?=w1922:bool)
                n1253 = Unflatten From String(type=T1 refnum ("New Image"), binary string=w1929, error in (no error)=errorcluster {"status"=FALSE, "code"=0, "source"=""}) -> (value=w1916:T1, error out=w1915:errorcluster)  [unwired: 3 out]
                n1254 = Select(t=errorcluster {"status"=FALSE, "code"=0, "source"=""}, s=w1922, f=w1921) -> (s? t:f=w1918:errorcluster)
                n1255 = case shown="No Error" w1915 {
                  tunnel: w1916 -> [w1938 _]
                  tunnel: [w1940 w1942] -> w1927
                  tunnel: w1928 -> [w1940 w1942]
                  tunnel: [w1938 w1941] -> w1926
                  tunnel: w1925 -> [_ w1941]
                  frame No Error {
                    n1256 = call "IMAQ Copy"("Image Dst"=w1940, "Image Src"=w1938) -> ("Image Dst Out"=→"Image Dst Out":T1)  [unwired: 4 in, 1 out]
                  }
                  frame Error {
                  }
                }
                n1257 = Unbundle By Name(w1918) -> ("status"=w1917:bool)
                n1258 = local read "restart"() -> (w1911:bool)
                n1259 = Compound Arithmetic op=OR(w1911, w1917) -> (w1936:bool)
              }
              n1260 = call "IMAQ Dispose"("Image"=w1905) -> ()  [unwired: 5 in, 1 out]
              n1261 = call "IMAQ Dispose"("Image"=w1906) -> ()  [unwired: 5 in, 1 out]
            }
          }
        }
        n1262 = local read "restart"() -> (w1892:bool)
      }
    }
    frame True {
    }
  }
  n1263 = stacked-sequence {
    frame #0 {
      n1264 = while {
        tunnel: [w1962] -> w1951
        tunnel: [w1960] -> w1950
        tunnel: [w1959] -> w1949
        tunnel: [w1958] -> w1948
        tunnel: [w1957] -> w1947
        tunnel: [w1956] -> w1946
        tunnel: [w1955] -> w1945
        tunnel: [w1954] -> w1944
        tunnel: [w1953] -> _
        tunnel: [w1952] -> w1943
        stop <- w1963 stop-if-true
        n1265 = local read "MirrorsNames"() -> (w1966:string[])
        n1266 = Empty Array?(array=w1966) -> (empty?=w1965:bool)
        n1267 = Not(x=w1965) -> (.not. x?=w1964:bool)
        n1268 = local read "stop"() -> (w1961:bool)
        n1269 = Or(x=w1964, y=w1961) -> (x .or. y?=w1963:bool)
        n1270 = Index Array(array=w1966) -> (element #1=w1962:string, element #2=w1960:string, element #3=w1959:string, element #4=w1958:string, element #5=w1957:string, element #6=w1956:string, element #7=w1955:string, element #8=w1954:string, element #9=w1953:string, element #10=w1952:string)  [unwired: 12 in, 2 out]
      }
      "GUIdevice 1" <- w1951
      "GUIdevice 2" <- w1950
      "GUIdevice 3" <- w1949
      "GUIdevice 4" <- w1948
      "GUIdevice 5" <- w1947
      "GUIdevice 6" <- w1946
      "GUIdevice 7" <- w1945
      "GUIdevice 8" <- w1944
      "GUIdevice 9" <- w1943
    }
    frame #1 {
      n1271 = Create User Event(user event datatype=T46 {"EventEnum"=enum."new data", "Device name"="Device name"} ("New Event")) -> (user event=w1968:refnum<user-event>, error out=w1969:errorcluster)  [unwired: 1 in]
      "tcp data event" <- w1968
      n1272 = control-ref of="This VI"() -> (w1972:refnum<vi>)
      n1273 = call "supergui create stop queue.vi"() -> ("STOP Queue out"=w1967:refnum<queue>)  [unwired: 11 in]
      n1274 = Current VI's Menubar() -> (w1971:refnum<k9>)
      n1275 = call "GUI_Master_subvi_reentrant_queues.vi"("STOP Queue in"=w1967, "error in (no error)"=w1969, "tcp data event"=w1968, "Caller menu reference"=w1971, "Caller VI ref"=w1972) -> ("error out"=→"error IO 2":errorcluster)  [unwired: 6 in]
    }
    frame #2 {
      n1276 = disable-structure shown="Enabled" {
        frame Enabled {
          n1277 = local write "MirrorsNames"(string[] [] ("MirrorsNames")) -> ()
        }
        frame Disabled {
        }
      }
    }
  }
  n1278 = local write "Main tab"(T18."User Main View" ("Main tab")) -> ()
  "image::1" <- T1 refnum ("New Image")
  "image::2" <- T1 refnum ("New Image")
  "image::3" <- T1 refnum ("New Image")
  "image::4" <- T1 refnum ("New Image")
  "image::5" <- T1 refnum ("New Image")
  "image::6" <- T1 refnum ("New Image")
  "image::7" <- T1 refnum ("New Image")
  "image::8" <- T1 refnum ("New Image")
  "image::9" <- T1 refnum ("New Image")
